vi "温度控制 - WK1.vi"(7 "CSM Name":string="WK1") -> ()   [LabVIEW 2026, in "UI-温度控制.lvlib"]
doc: "本范例执行串口读写操作。串口设置的参数必须匹配连接仪器或设备的参数。“VISA配置串口”VI可设置配置参数。前面板显示的控件可用于配置基本参数，如波特率、数据位和校验。VI会将VISA资源名称传递至其他VI以便执行相关操作。“VISA写入”函数将发送一个命令至串行设备，“VISA读取”函数将返回基于该命令的数据。“VISA关闭”函数可关闭该串行设备的引用。关闭引用十分重要，否则可能导致无法通过该端口进行进一步通信。"
uses:
  Supports/Sample Settings.ctl
  Data ColndSave/Supports/Time and Data.ctl
  Supports/Device Info.ctl
  Supports/Repeat Steps.ctl
  <userlib>/_NEVSTOP/Communicable State Machine(CSM)/_Polymophic/CSM - Filter Duplicated Lines.vi
  <userlib>/_NEVSTOP/Communicable State Machine(CSM)/_Polymophic/Add State(s) to Queue By BOOL(Element).vi
  e87f5527-76ec-45cd-8a15-2e3ba2958834.vi
  e40b3fcb-6c9f-41ae-97ff-bcb9991e0652.vi
  620e82e9-b677-4d25-b56c-4b090e123e3d.vi
  fecb341a-c865-4baa-9917-6b90415d6ef9.vi
  afd7753c-ea30-4e5b-9716-29bc73ab5d02.vi
  9a199716-2ffa-4f43-b9de-bb583d0dc84c.vi
  b5fe0464-1048-4df8-950b-6816aac68042.vi
  026bd4a5-6a46-4a68-819b-9f168641a175.vi
  3bdb7142-561a-47bb-abd8-0318bec92597.vi
  36fd150c-2ad9-4592-a276-8ca334c7aa56.vi
  6094d1ba-01c9-4f0f-81c2-2bfc5faa83cd.vi
  6f01d93e-47d7-4c16-bfcb-79e48a01ebec.vi
  f347ec19-a9ab-456c-bf02-8d1d7c992b68.vi
  b7989555-3743-433e-92bc-1f24cc67f5f4.vi
  9b669b8c-733c-4058-8ee2-0fdaa3bce225.vi
  7ceba0d5-fd35-45f6-9e4f-db13be910fa9.vi
  e0d25892-2f3c-4bdd-91b3-ce78b04bde2a.vi
  e709ab76-91cd-483a-bfeb-5221a7f7e432.vi
  6fdd3ccc-b7af-4740-b642-363912b39baa.vi
  52a88361-96b9-4f42-83b5-2b3a91f6fe46.vi
  <userlib>/_NEVSTOP/Communicable State Machine(CSM)/_Polymophic/CSM - Replace Marks in Messages.vi
  3eee923a-0692-424c-8c25-dbf31775acba.vi
  7f493404-46e2-4a42-937c-85a599ffd008.vi
  e181f527-371e-42fd-b1ab-20e25477ecf6.vi
  3c0606d2-39f9-4349-a74d-1248628ec5a5.vi
  2a5f06fa-bc14-4be7-8a56-d3603e987429.vi
  b1075206-a0bc-4c2c-8117-03daddfb89bc.vi
  f1339c31-251d-401b-9b2c-5eea904d101d.vi
  12798cb0-d503-413b-8ceb-4a5576430bcb.vi
  342b248c-6441-4aa8-8129-3c8b576c20b5.vi
  bd3fa8c0-2a07-4348-928a-5492c50b8d1d.vi
  bfd69444-e477-482d-b4ce-b6780147d2f5.vi
  22b4bb12-f94e-4276-9d0b-49463fdbebaf.vi
  87263e8e-d87a-4015-b0d9-f89f6746087b.vi
  45ac6a38-59b2-4408-864e-de2893445c95.vi
  3f8d9458-3e99-4457-8efa-55d1ef2330f2.vi
  bd3177e1-6bd6-42ad-a258-ed35146a2f34.vi
  acea6df9-f425-4d5c-b033-3243991d638c.vi
  611bdd8b-2aca-4a53-81a9-536b5b4081e0.vi
  6c66f1b3-0c4e-481a-bccf-761e4204c7a2.vi
  69110340-9523-4369-a866-1e083b49cebd.vi
  dc7ef564-96da-43a3-866d-645d9c897f58.vi
  cab45986-ae3d-44a0-b15a-916822da0a04.vi
  6e92e572-67e2-4f23-93e9-3f2621f8ebb2.vi
  fcc43e12-244c-4800-bcec-4b40395c6c4b.vi
  b77c82fb-bb1b-4fca-94e8-a2470f067fd9.vi
  <userlib>/_NEVSTOP/Communicable State Machine(CSM)/AdvanceAPI/CSM - Compact Multiple States.vi
  <userlib>/_NEVSTOP/Communicable State Machine(CSM)/AdvanceAPI/CSM - Break Down Multiple States String.vi
  <userlib>/_NEVSTOP/Communicable State Machine(CSM)/_Shared/Remove Comments from Single-line.vi
  <userlib>/_NEVSTOP/Communicable State Machine(CSM)/_Shared/Split Single-line Message.vi
  <userlib>/_NEVSTOP/Communicable State Machine(CSM)/_Shared/Trim Single-line Text.vi
  <userlib>/_NEVSTOP/Communicable State Machine(CSM)/_Shared/Add State(s) to Queue__jkism.vi
  <userlib>/_NEVSTOP/Communicable State Machine(CSM)/AdvanceAPI/CSM - Revert Arguments-Safe String.vi
  <userlib>/_NEVSTOP/Communicable State Machine(CSM)/AdvanceAPI/CSM - Make String Arguments Safe.vi
  e709ab76-91cd-483a-bfeb-5221a7f7e432.vi/99de0c97-112a-4c86-9094-c187659127e1.vi
  <userlib>/_NEVSTOP/Communicable State Machine(CSM)/Utility/Build Error Cluster.vi
  52a88361-96b9-4f42-83b5-2b3a91f6fe46.vi/99de0c97-112a-4c86-9094-c187659127e1.vi
  cab45986-ae3d-44a0-b15a-916822da0a04.vi/b09b9099-6be0-413b-8afc-4908471460c3.vi
  <userlib>/_NEVSTOP/Communicable State Machine(CSM)/addons/INI-Static-Variable-Support/_Support/FlagInstance-CSMINIVariable.vi
  b77c82fb-bb1b-4fca-94e8-a2470f067fd9.vi/99de0c97-112a-4c86-9094-c187659127e1.vi
  <vilib>/Utility/error.llb/Trim Whitespace.vi
  <vilib>/Utility/error.llb/Trim Whitespace (string).vi
  <userlib>/_NEVSTOP/Communicable State Machine(CSM)/AdvanceAPI/CSM - Keywords.vi
  <userlib>/_NEVSTOP/Communicable State Machine(CSM)/_Support/ChangeFlag/ChangeFlag-Read.vi
  <vilib>/Utility/error.llb/Trim Whitespace One-Sided.vi
  <userlib>/_NEVSTOP/Communicable State Machine(CSM)/addons/API-String-Arugments-Support/_Support/Data To API String Arguments.vi
  <userlib>/_NEVSTOP/Communicable State Machine(CSM)/addons/INI-Static-Variable-Support/_Support/instances/_CSM - Read File Logger Configuration - v1.0.vi
  <vilib>/Utility/Data Type/Get Type Information.vi
  <userlib>/_NEVSTOP/Communicable State Machine(CSM)/addons/API-String-Arugments-Support/_Support/Data To SingleElementsArray_csm.vi
  <userlib>/_NEVSTOP/Communicable State Machine(CSM)/addons/INI-Static-Variable-Support/_Support/Parse Used Session and Name.vi
  <userlib>/_NEVSTOP/Communicable State Machine(CSM)/addons/INI-Static-Variable-Support/_Support/INI-FGV(lvlibp).vi
  <userlib>/_NEVSTOP/Communicable State Machine(CSM)/addons/INI-Static-Variable-Support/_Support/Populate String with INI Variable.vi
  <userlib>/_NEVSTOP/Communicable State Machine(CSM)/addons/API-String-Arugments-Support/_Support/Convert API String Arguments to Data(variant).vi
  <userlib>/_NEVSTOP/Communicable State Machine(CSM)/addons/API-String-Arugments-Support/_Support/SingleElementsArray To Data_csm.vi
  <userlib>/_NEVSTOP/Communicable State Machine(CSM)/addons/MassData-Parameter/_support/FGV-MassData(lvlibp).vi
  <vilib>/Instr/_visa.llb/VISA Configure Serial Port (Instr).vi
  Repeat/Repeat.vi
  <userlib>/_NEVSTOP/Communicable State Machine(CSM)/_Support/ChangeFlag/ChangeFlagDB.vi
  <userlib>/_NEVSTOP/Communicable State Machine(CSM)/Communicable State Machine.lvlib
  <userlib>/_NEVSTOP/Communicable State Machine(CSM)/addons/MassData-Parameter/CSM MassData Parameter Support.lvlib
  <userlib>/_NEVSTOP/Communicable State Machine(CSM)/addons/INI-Static-Variable-Support/INI-Static-Variable-Support.lvlib
  <userlib>/_NEVSTOP/Communicable State Machine(CSM)/addons/Watchdog/CSM Watchdog.lvlib
  <userlib>/_NEVSTOP/Communicable State Machine(CSM)/addons/Logger/CSM File Logger.lvlib
  Logging/Logging.lvlib
  Repeat/Repeat.lvlib
  b63380f4-522f-43f9-8c86-ff87e18121f1.vi
  Acquisition/Acquisition.lvlib
  Data ColndSave/Data Collection and Save.lvlib
panel:
  in  "停止":bool
  in  "温度显示":T1(tab)
  in  "下限 2":dbl=25.0 min=-10.0 max=50.0 step=0.1 format="%.1g"
  in  "上限 2":dbl=25.0 min=-10.0 max=50.0 step=0.1 format="%.1g"
  in  "下限 1":dbl=25.0 min=-10.0 max=50.0 step=0.1 format="%.1g"
  in  "上限 1":dbl=25.0 min=-10.0 max=50.0 step=0.1 format="%.1g"
  in  "温控开关 总":bool
  in  "跟随通道 1":T2
  in  "跟随通道 2":T2
  in  "通道":bool
  in  "温控温度 B":dbl=25.0 min=-10.0 max=50.0 step=0.1 format="%.2g"
  in  "温控温度 A":dbl=25.0 min=-10.0 max=50.0 step=0.1 format="%.2g"
  in  "温度":bool
  in  "跟随偏移 2":dbl min=-10.0 max=50.0 step=0.01 format="%#.2g"
  in  "是否跟随 2":bool
  in  "跟随偏移 1":dbl min=-10.0 max=50.0 step=0.01 format="%#.2g"
  in  "是否跟随 1":bool
  in  "打开串口":bool
  in  "温控串口":refnum<visa-resource-name>="COM18"
  out "TC2":waveform(dbl)[](graph)
  out "TC1":waveform(dbl)[](graph)
  in  "温控开关 2":bool
  in  "温控开关 1":bool
  in  "温控温度 2":dbl=25.0 min=-10.0 max=50.0 step=0.1 format="%.2g"
  out "实际温度 2":dbl=25.0 format="%.2g"
  out "实际温度 1":dbl=25.0 format="%.2g"
  in  "温控温度 1":dbl=25.0 min=-10.0 max=50.0 step=0.1 format="%.2g"
  in  "Fast Mode":bool
  in  "采集间隔":dbl=0.5 min=0.05 max=50.0 step=0.1 format="%.2g"
  out "Power 2":waveform(dbl)[](graph)
  out "Power 1":waveform(dbl)[](graph)
  out "输出状态 1":T3
  out "输出状态 2":T3
  in  "电源切换 2":bool
  in  "电源切换 1":bool
  in  "输出设置 2":T4={"输出模式"=enum."加热模式", "最大输出电压"=5.0} {"最大输出电压" min=0.0001 max=10.0 format="%.1g"}
  in  "输出设置 1":T4={"输出模式"=enum."加热模式", "最大输出电压"=5.0} {"最大输出电压" min=0.0001 max=10.0 format="%.1g"}
  in  "PID 1":T5={"PID类型"=enum."PID", "P"=0.05, "I"=20.0, "D"=2.0, "PID控制间隔"=100.0, "PID计算方法"=enum."最大正向输出"}
  in  "PID 2":T5={"PID类型"=enum."PID", "P"=0.05, "I"=20.0, "D"=2.0, "PID控制间隔"=100.0, "PID计算方法"=enum."最大正向输出"}
  in  "过压/过流 2":cluster{"过压保护阈值":dbl, "过流保护阈值":dbl}={"过压保护阈值"=6.0, "过流保护阈值"=3.0}
  in  "过压/过流 1":cluster{"过压保护阈值":dbl, "过流保护阈值":dbl}={"过压保护阈值"=6.0, "过流保护阈值"=3.0}
  in  "过温 2":T6={"过温保护开关"=TRUE, "过温保护低阈值"=5.0, "过温保护高阈值"=45.0, "最低设定温度"=5.0, "最高设定温度"=45.0, "温度限速"=45.0} {"温度限速" min=0.01}
  out "保护结果 2":T7={"过压保护结果"=enum."正常", "过流保护结果"=enum."正常", "过温保护结果"=enum."正常"}
  out "保护结果 1":T7={"过压保护结果"=enum."正常", "过流保护结果"=enum."正常", "过温保护结果"=enum."正常"}
  in  "过温 1":T6={"过温保护开关"=TRUE, "过温保护低阈值"=5.0, "过温保护高阈值"=45.0, "最低设定温度"=5.0, "最高设定温度"=45.0, "温度限速"=45.0} {"温度限速" min=1e-06; "最低设定温度" min=0.0001}
  in  "温控循环功能":bool
  in  "子程序？":bool
  out "温控-错误输出":errorcluster
  out "温控器设备型号":string
  out "State History":string
  # "温度快切"
  # "V"
  # "A"
  # "V"
  # "A"
  # "V"
  # "V"
  # "ms"
  # "ms"
  # "℃/s"
  # "℃/s"
  # "恢复，继续运行；\n如继续报错，请检查参数，可尝试关闭串口重新打开。"
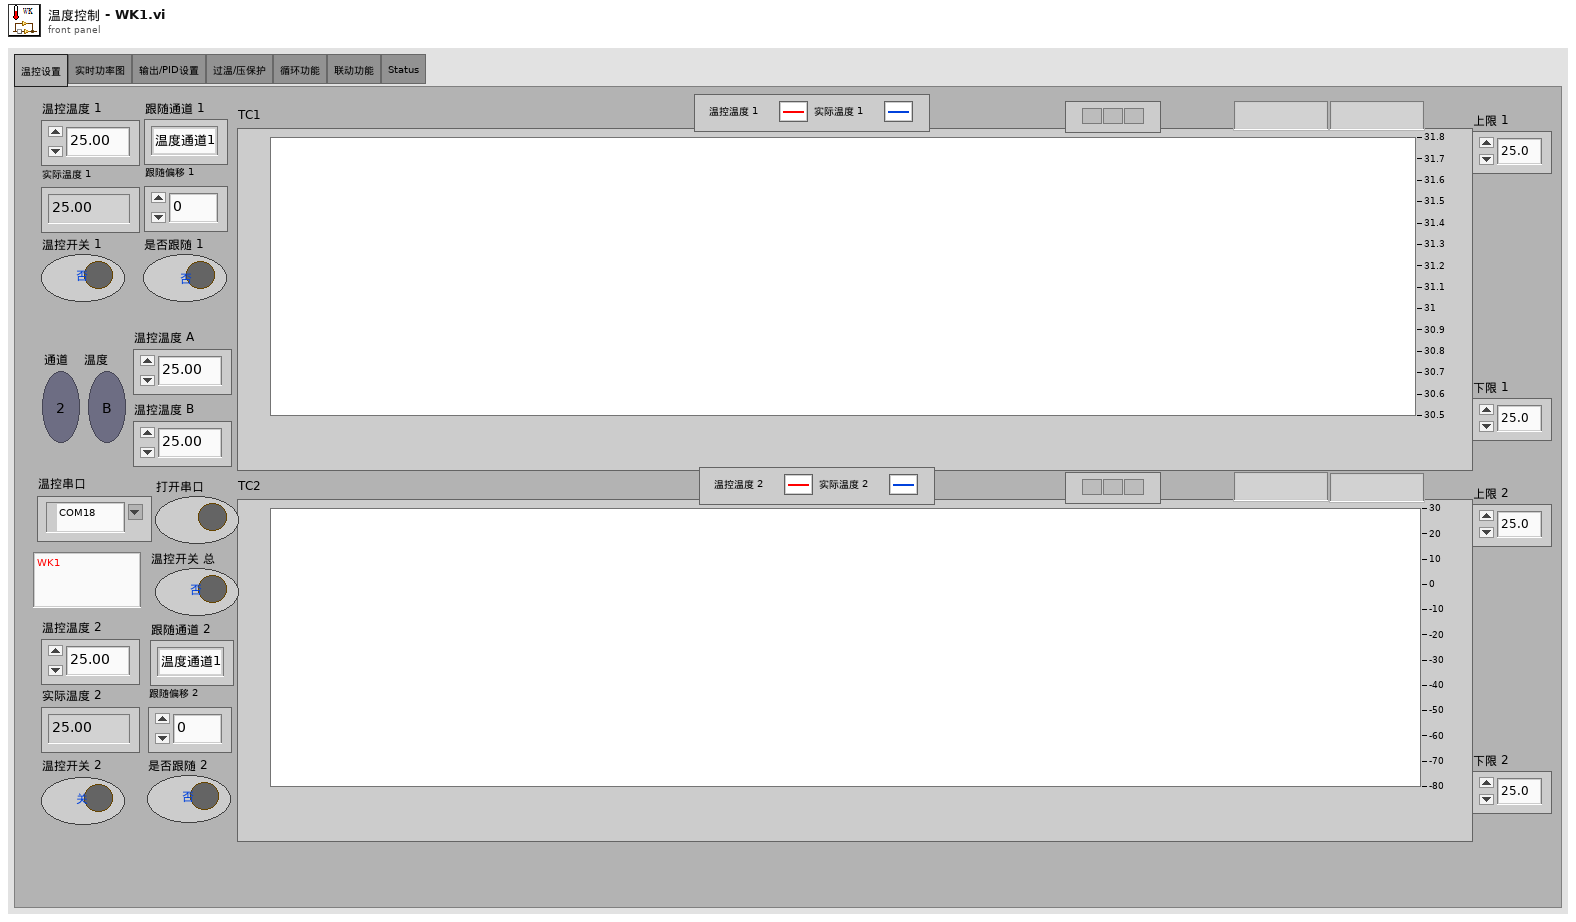
[diagram p1: front panel]
types:
  T1 = enum32{"温控设置", "实时功率图", "输出/PID设置", "过温/压保护", "循环功能", "联动功能", "Status"}
  T2 = typedef "温度通道索引_全局.ctl" = enum16{"温度通道1", "温度通道2", "温度通道3", "温度通道4", "温度通道5", "温度通道6", "温度通道7", "温度通道8", "TC1控制温度", "TC1实际温度", "TC1实际输出电压", "TC1实际输出电流", "TC1实际输出功率", "TC2控制温度", "TC2实际温度", "TC2实际输出电压", "TC2实际输出电流", "TC2实际输出功率", "压力(电压值)", "压力(g)", "Zolix当前位置", "Zolix速度", "步进电机位置", "步进电机速度", "温度", "湿度"}
  T3 = cluster{"功率输出":enum16{"已关闭", "已打开"}, "实际输出电压":dbl, "实际输出电流":dbl}
  T4 = cluster{"输出模式":enum16{"致冷模式", "加热模式", "双向模式"}, "最大输出电压":dbl}
  T5 = cluster{"PID类型":enum16{"P", "PI", "PID"}, "P":dbl, "I":dbl, "D":dbl, "PID控制间隔":dbl, "PID计算方法":enum16{"位置式", "增量式", "最大正向输出", "最大负向输出"}}
  T6 = cluster{"过温保护开关":bool, "过温保护低阈值":dbl, "过温保护高阈值":dbl, "最低设定温度":dbl, "最高设定温度":dbl, "温度限速":dbl}
  T7 = cluster{"过压保护结果":enum16{"发现错误", "正常", "功能关闭"}, "过流保护结果":enum16{"发现错误", "正常", "功能关闭"}, "过温保护结果":enum16{"发现错误", "正常", "功能关闭"}}
  T8 = cluster{"Enable":bool, "Limit":cluster{"FileSize":i64, "FileNum":i32}, "Timestamp.Format":string, "AutoExit":bool}
  T9 = enum32{"Invalid", "Standard", "Closed", "Hidden", "Minimized", "Maximized"}
  T10 = enum32{"invalid app kind", "Development System", "Run Time System", "Student Edition", "Embedded LabVIEW", "Evaluation", "Custom"}
  T11 = typedef "UI-温度控制.lvlib/Device Info.ctl" = cluster{"基本信息":cluster{"USB Port":refnum<visa-resource-name>, "采集间隔(s)":dbl}, "设备信息":cluster{"设备型号":string, "双通道设备？":bool}, "开关":cluster{"开关 1":bool, "开关 2":bool, "Fast Mode":bool}, "Control Temp":cluster{"Control Temp 1":dbl, "Control Temp 2":dbl}}
  T12 = cluster{"波特率":u32, "数据位":u16, "校验":enum16{"None", "Odd", "Even", "Mark", "Space"}, "停止位":u16, "流控制":u16}
  T13 = typedef "Communicable State Machine.lvlib/_CSM_Response Source Message.ctl" = cluster{"‘State":string, "’Arguments":string, "’Error":errorcluster}
  T14 = cluster{"Current VI Reference":refnum<vi>, "Close Panel on Exit?":bool}
  T15 = typedef "UI-温度控制.lvlib/Sample Settings.ctl" = cluster{"USB Port":refnum<visa-resource-name>, "采集间隔(s)":dbl}
  T16 = typedef "Data Collection and Save.lvlib/Time and Data.ctl" = cluster{"采集时间":timestamp, "Data":dbl[]}
  T17 = cluster{"Core":cluster{"Current VI Reference":refnum<vi>, "Close Panel on Exit?":bool}, "基本信息":T15, "温控情况":cluster{"温控温度 1":dbl, "实际温度 1":dbl, "温控温度 2":dbl, "实际温度 2":dbl, "打开串口":bool}, "开关信息":cluster{"开关 1":bool, "开关 2":bool, "温控是否打开":bool}, "输出参数":cluster{"输出设置 1":cluster{"输出模式":enum16{"致冷模式", "加热模式", "双向模式"}, "最大输出电压":dbl}, "输出设置 2":cluster{"输出模式":enum16{"致冷模式", "加热模式", "双向模式"}, "最大输出电压":dbl}, "输出状态 1":cluster{"功率输出":enum16{"已关闭", "已打开"}, "实际输出电压":dbl, "实际输出电流":dbl, "实际输出功率":dbl}, "输出状态 2":cluster{"功率输出":enum16{"已关闭", "已打开"}, "实际输出电压":dbl, "实际输出电流":dbl, "实际输出功率":dbl}, "PID 1":cluster{"PID类型":enum16{"P", "PI", "PID"}, "P":dbl, "I":dbl, "D":dbl, "PID控制间隔":dbl, "PID计算方法":enum16{"位置式", "增量式", "最大正向输出", "最大负向输出"}}, "PID 2":cluster{"PID类型":enum16{"P", "PI", "PID"}, "P":dbl, "I":dbl, "D":dbl, "PID控制间隔":dbl, "PID计算方法":enum16{"位置式", "增量式", "最大正向输出", "最大负向输出"}}}, "保护":cluster{"过压/过流 1":cluster{"过压保护阈值":dbl, "过流保护阈值":dbl}, "过压/过流 2":cluster{"过压保护阈值":dbl, "过流保护阈值":dbl}, "保护结果 1":cluster{"过压保护结果":enum16{"发现错误", "正常", "功能关闭"}, "过流保护结果":enum16{"发现错误", "正常", "功能关闭"}, "过温保护结果":enum16{"发现错误", "正常", "功能关闭"}}, "保护结果 2":cluster{"过压保护结果":enum16{"发现错误", "正常", "功能关闭"}, "过流保护结果":enum16{"发现错误", "正常", "功能关闭"}, "过温保护结果":enum16{"发现错误", "正常", "功能关闭"}}, "过温 1":cluster{"过温保护开关":bool, "过温保护低阈值":dbl, "过温保护高阈值":dbl, "最低设定温度":dbl, "最高设定温度":dbl, "温度限速":dbl}, "过温 2":cluster{"过温保护开关":bool, "过温保护低阈值":dbl, "过温保护高阈值":dbl, "最低设定温度":dbl, "最高设定温度":dbl, "温度限速":dbl}}, "设备信息":cluster{"设备型号":string, "双通道设备？":bool}, "Time and Data":T16, "其他":cluster{"子程序？":bool, "Fast Mode?":bool, "Auto Range 1?":bool, "Auto Range 2?":bool}}
  T18 = cluster{"子程序？":bool, "Fast Mode?":bool, "Auto Range 1?":bool, "Auto Range 2?":bool}
  T19 = cluster{"过压/过流 1":cluster{"过压保护阈值":dbl, "过流保护阈值":dbl}, "过压/过流 2":cluster{"过压保护阈值":dbl, "过流保护阈值":dbl}, "保护结果 1":cluster{"过压保护结果":enum16{"发现错误", "正常", "功能关闭"}, "过流保护结果":enum16{"发现错误", "正常", "功能关闭"}, "过温保护结果":enum16{"发现错误", "正常", "功能关闭"}}, "保护结果 2":cluster{"过压保护结果":enum16{"发现错误", "正常", "功能关闭"}, "过流保护结果":enum16{"发现错误", "正常", "功能关闭"}, "过温保护结果":enum16{"发现错误", "正常", "功能关闭"}}, "过温 1":cluster{"过温保护开关":bool, "过温保护低阈值":dbl, "过温保护高阈值":dbl, "最低设定温度":dbl, "最高设定温度":dbl, "温度限速":dbl}, "过温 2":cluster{"过温保护开关":bool, "过温保护低阈值":dbl, "过温保护高阈值":dbl, "最低设定温度":dbl, "最高设定温度":dbl, "温度限速":dbl}}
  T20 = cluster{"输出设置 1":cluster{"输出模式":enum16{"致冷模式", "加热模式", "双向模式"}, "最大输出电压":dbl}, "输出设置 2":cluster{"输出模式":enum16{"致冷模式", "加热模式", "双向模式"}, "最大输出电压":dbl}, "输出状态 1":cluster{"功率输出":enum16{"已关闭", "已打开"}, "实际输出电压":dbl, "实际输出电流":dbl, "实际输出功率":dbl}, "输出状态 2":cluster{"功率输出":enum16{"已关闭", "已打开"}, "实际输出电压":dbl, "实际输出电流":dbl, "实际输出功率":dbl}, "PID 1":cluster{"PID类型":enum16{"P", "PI", "PID"}, "P":dbl, "I":dbl, "D":dbl, "PID控制间隔":dbl, "PID计算方法":enum16{"位置式", "增量式", "最大正向输出", "最大负向输出"}}, "PID 2":cluster{"PID类型":enum16{"P", "PI", "PID"}, "P":dbl, "I":dbl, "D":dbl, "PID控制间隔":dbl, "PID计算方法":enum16{"位置式", "增量式", "最大正向输出", "最大负向输出"}}}
  T21 = cluster{"温控温度 1":dbl, "实际温度 1":dbl, "温控温度 2":dbl, "实际温度 2":dbl, "打开串口":bool}
  T22 = enum8{"Enabled", "Disabled", "Disabled and Grayed Out"}
  T23 = typedef "UI-温度控制.lvlib/Repeat Steps.ctl" = cluster{"控制温度":dbl, "时长(s)":dbl, "进度":dbl, "温控开关":bool}[]
  T24 = cluster{"PID类型":bool, "P":bool, "I":bool, "D":bool, "PID控制间隔":bool, "PID计算方法":bool}
  T25 = cluster{"过温保护开关":bool, "过温保护低阈值":bool, "过温保护高阈值":bool, "最低设定温度":bool, "最高设定温度":bool, "温度限速":bool}
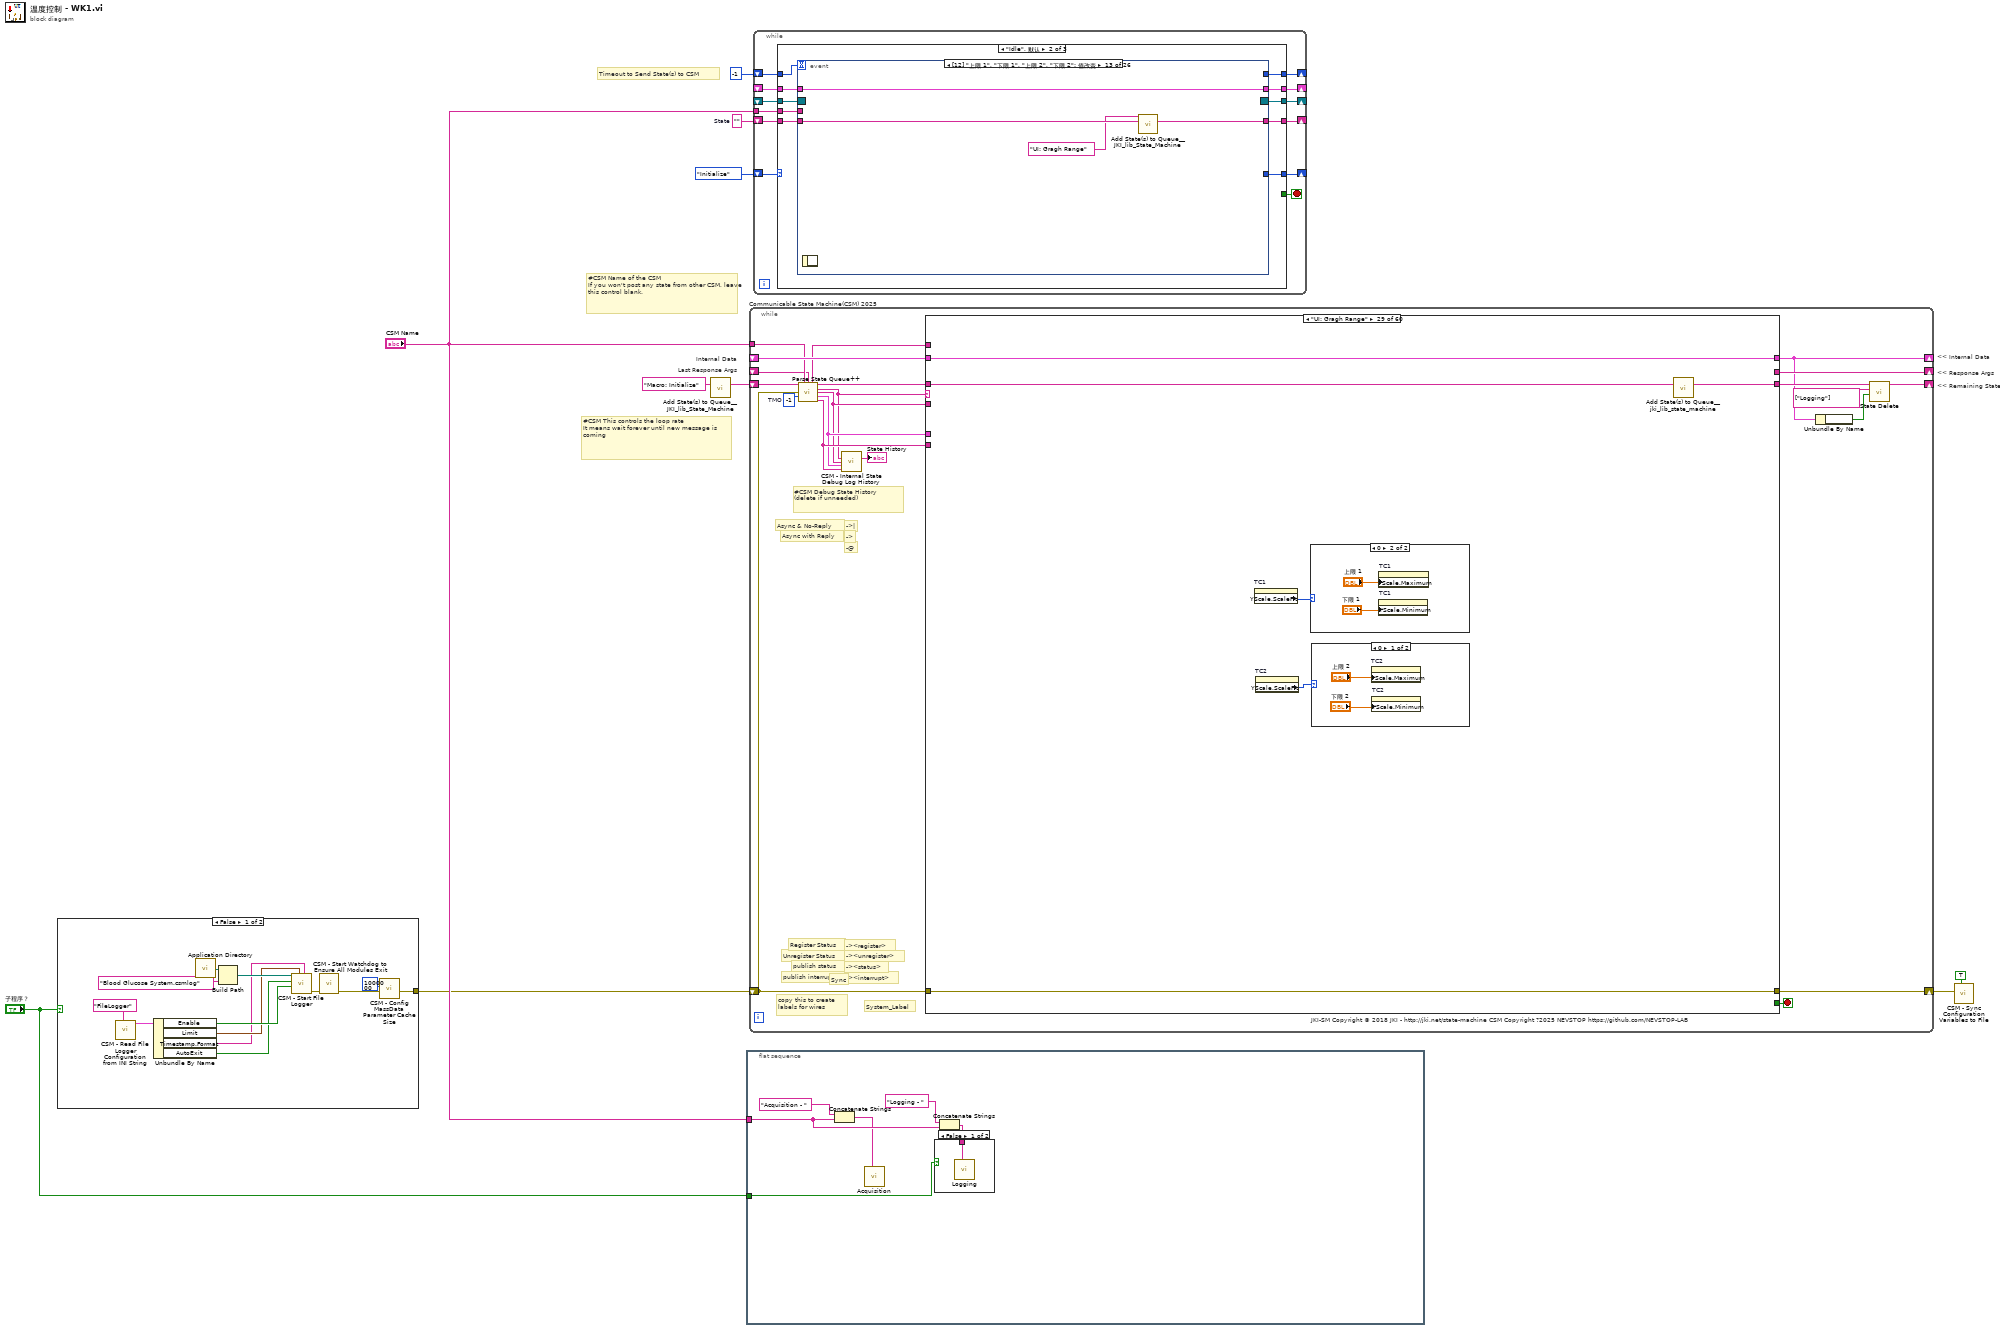
[diagram p0: block diagram]
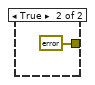
[diagram p2: hidden frame]
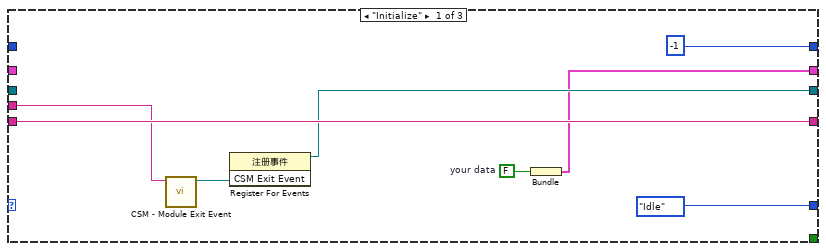
[diagram p4: hidden frame]
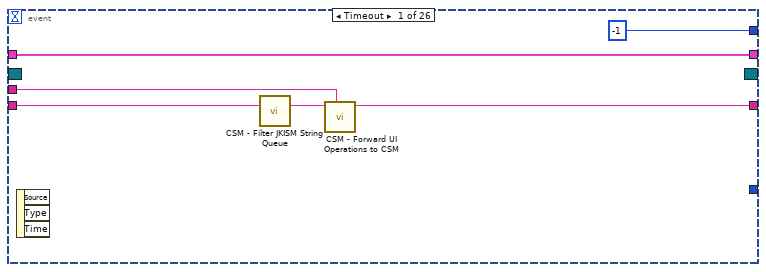
[diagram p5: hidden frame]
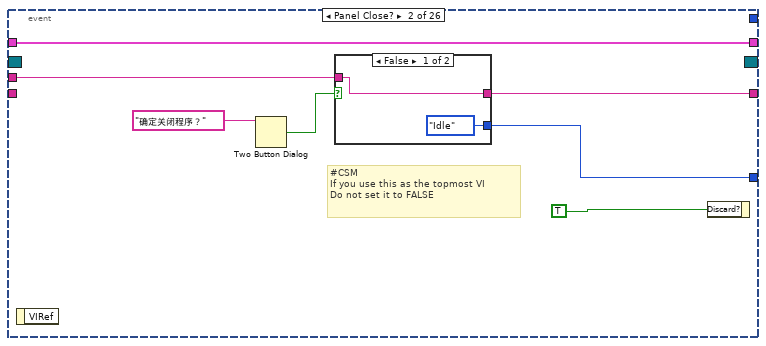
[diagram p6: hidden frame]
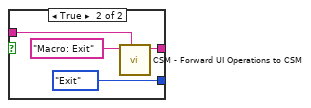
[diagram p7: hidden frame]
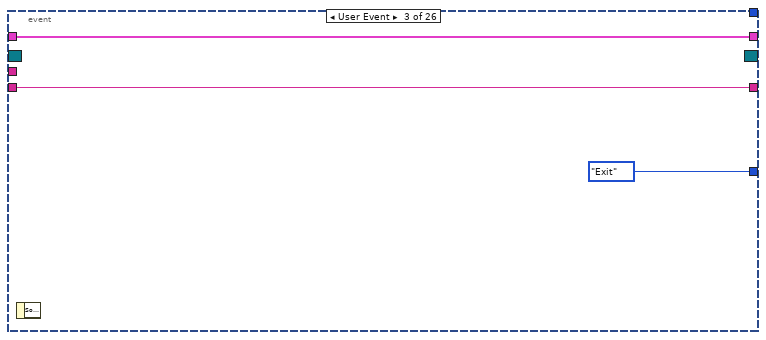
[diagram p8: hidden frame]
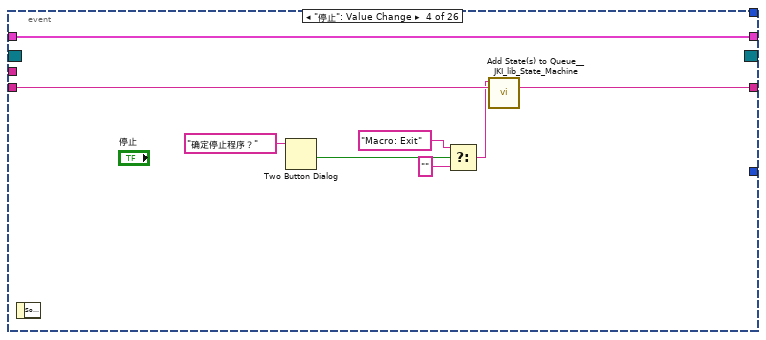
[diagram p9: hidden frame]
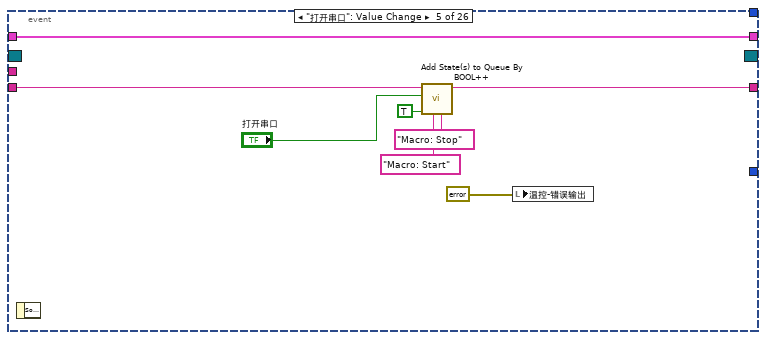
[diagram p10: hidden frame]
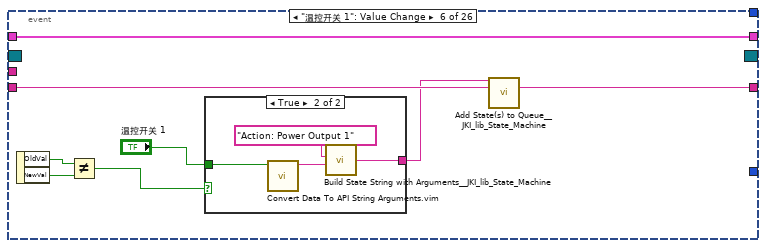
[diagram p11: hidden frame]
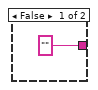
[diagram p12: hidden frame]
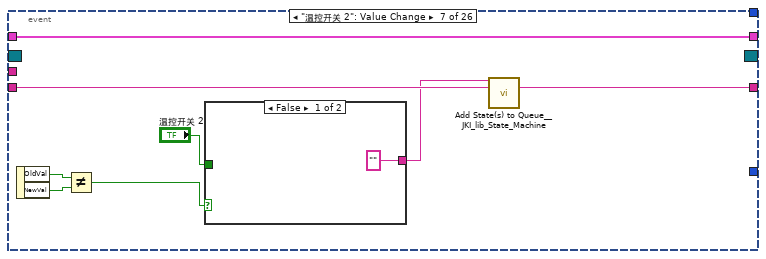
[diagram p13: hidden frame]
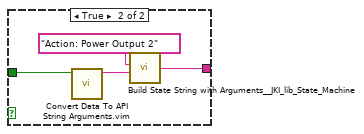
[diagram p14: hidden frame]
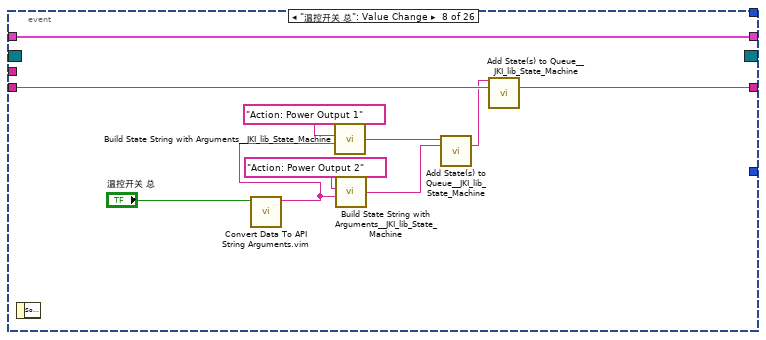
[diagram p15: hidden frame]
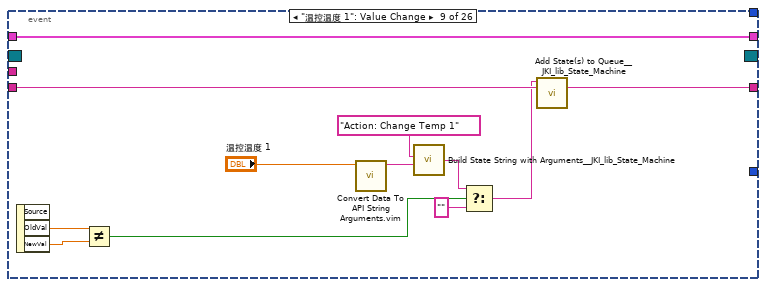
[diagram p16: hidden frame]
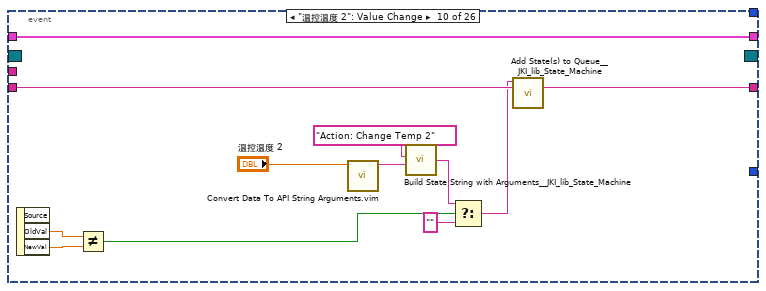
[diagram p17: hidden frame]
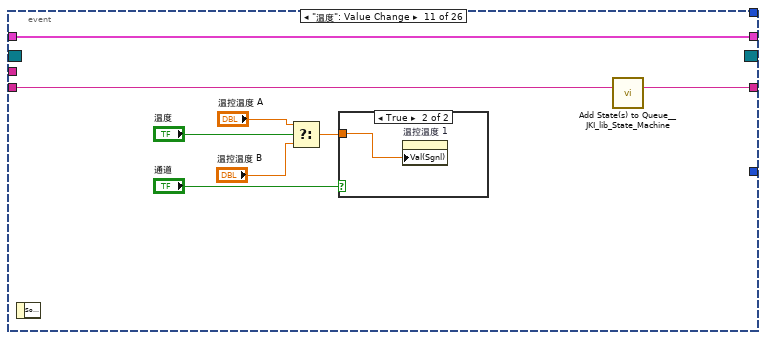
[diagram p18: hidden frame]
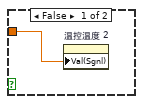
[diagram p19: hidden frame]
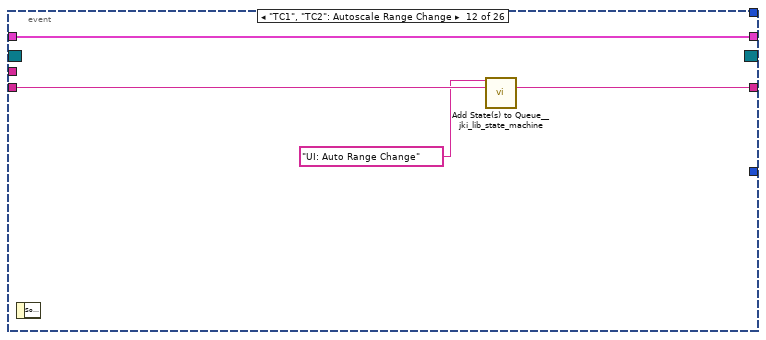
[diagram p20: hidden frame]
diagram:
  w9 = ""  # State
  # "Timeout to Send State(s) to CSM"
  # "Last Response Args"
  # "Internal Data"
  # "#CSM Name of the CSM\nIf you won't post any state from other CSM, leave this control blank."
  # "#CSM This controls the loop rate\nIt means wait forever until new message is coming"
  # "<< Internal Data"
  # "<< Response Args"
  # "<< Remaining States"
  n1 = case shown="False" "子程序？" {
    tunnel: [w21 errorcluster {"status"=FALSE, "code"=0, "source"=""} ("Error out")] -> w2
    frame False {
      n2 = call-poly <userlib>:"CSM - Read File Logger Configuration from INI String.vi"("Section Name(\"FileLogger\")"="FileLogger" ("Section Name(\"\" as Default)")) -> ("FileLogger Configuration-v1"=w15:T8)  [unwired: 7 in, 1 out]
      n3 = Unbundle By Name(w15) -> ("Enable"=w14:bool, "Limit"=w13:cluster{"FileSize":i64, "FileNum":i32}, "Timestamp.Format"=w11:string, "AutoExit"=w12:bool)
      n4 = call <vilib>:"Application Directory.vi"() -> ("Application Directory"=w20:path)
      n5 = Build Path(base path=w20, name or relative path="Blood Glucose System.csmlog") -> (appended path=w18:path)
      n6 = call <userlib>:"CSM - Start File Logger.vi"("Timestamp Format"=w11, "Log Limit"=w13, "Watchdog? (T)"=w14, "Exit When All Module Exist? (F)"=w12, "Log File Path"=w18) -> ("error out"=w17:errorcluster)  [unwired: 4 in, 2 out]
      n7 = call <userlib>:"CSM - Start Watchdog to Ensure All Modules Exit.vi"("error in (no error)"=w17) -> ("error out"=w22:errorcluster)  [unwired: 10 in]
      n8 = call <userlib>:"CSM - Config MassData Parameter Cache Size.vi"("Error in"=w22, "Size (50M)"=1000000 ("size(1M)")) -> ("Error out"=w21:errorcluster)  [unwired: 9 in]
    }
    frame True {
    }
  }
  n9 = call <vilib>:"Add State(s) to Queue__JKI_lib_State_Machine.vi"("State(s) in (\"\")"="Macro: Initialize" ("Init State(\"Macro: Initialize\")")) -> ("States Out"=w6:string)  [unwired: 14 in]
  n10 = flat-sequence {
    tunnel: "CSM Name" -> [w27]
    tunnel: "子程序？" -> [w25]
    frame #0 {
      n11 = Concatenate Strings("Acquisition - " ("Name(\"\" to use uuid)"), w27) -> (w26:string)
      n12 = call "Acquisition.vi"("CSM Name"=w26) -> ()  [unwired: 11 in]
      n13 = Concatenate Strings("Logging - " ("Name(\"\" to use uuid)"), w27) -> (w28:string)
      n14 = case shown="False" w25 {
        tunnel: w28 -> [w31 _]
        frame False {
          n15 = call "Logging.vi"("CSM Name"=w31) -> ()  [unwired: 11 in]
        }
        frame True {
        }
      }
    }
  }
  n16 = while "Communicable State Machine(CSM) 2025" {
    shift-right: [w33] -> _
    shift-left: _ -> [w48]
    shift-right: [w50] -> w4
    shift-left: w2 -> [w39]
    shift-right: [w35] -> _
    shift-left: w6 -> [w51]
    tunnel: "CSM Name" -> [w45]
    shift-right: [w46] -> _
    shift-left: _ -> [w40]
    stop <- w49 stop-if-true
    w47 = -1  # TMO
    # "#CSM Debug State History\n(delete if unneeded)"
    # "-><interrupt>"
    # "-><status>"
    # "-><unregister>"
    # "-><register>"
    # "-@"
    # "->"
    # "->|"
    # "publish interrupt"
    # "publish status"
    # "Unregister Status"
    # "Register Status"
    # "Sync"
    # "Async with Reply"
    # "Async & No-Reply"
    # "JKI-SM Copyright © 2018 JKI - http://jki.net/state-machine CSM Copyright ?2025 NEVSTOP https://github.com/NEVSTOP-LAB"
    # "copy this to create labels for wires"
    # "System_Label"
    n17 = call <userlib>:"Parse State Queue++.vi"("State Queue"=w51, "Name (\"\" to Use UUID)"=w45, "Response Arguments"=w40, "Previous Error"=w39, "Dequeue (1 ms)"=w47) -> ("Name Used"=w37:string, "Remaining States"=w52:string, "Current State"=w41:string, "Arguments"=w42:string, "Additional Information"=w43:T13, "Source CSM"=w44:string)  [unwired: 5 in]
    n18 = call <userlib>:"CSM - Internal State Debug Log History.vi"("State"=w41, "Arguments (\"\")"=w42, ">> Response Source Message >>"=w43, "Source (\"\")"=w44) -> ("Debug Log"=→"State History":string)  [unwired: 11 in]
    n19 = case shown="\"UI: Gragh Range\"" w41 {
      selector: w41 -> [_ _ _ w64 _ _ _ _ _ _ _ _ _ _ _ _ _ _ _ _ _ _ _ _ _ _ _ _ _ _ _ _ _ _ _ _ _ _ _ _ _ _ _ _ _ _ _ _ _ _ _ _ _ _ _ _ _ _ _ _]
      tunnel: w52 -> [w53 w57 w60 w68 w73 w79 w104 w110 w116 w126 w133 w145 w149 w152 w172 w212 w238 w240 w261 w263 w295 w321 w352 w383 w440 w514 w546 w553 w558 w567 w573 w619 w632 w661 w673 w676 w694 w712 w737 w749 w788 w803 w812 w839 w869 w914 w959 w1005 w1051 w1080 w1099 w1106 w1112 w1120 w1133 w1140 w1153 w1166 w1178 w1183]
      tunnel: w42 -> [_ _ _ _ _ w78 w100 w107 w113 w120 _ _ _ _ _ w205 _ _ _ _ _ _ _ _ _ _ _ _ _ _ _ _ _ _ _ _ w686 w704 w726 w743 w781 w796 w811 w838 w868 w913 w958 w1004 w1050 w1079 _ w1104 w1115 w1123 w1130 _ _ w1164 _ _]
      tunnel: w48 -> [w55 w56 w58 w66 w72 w84 w102 w108 w114 w124 w132 w139 w147 w150 _ w183 w233 w241 w245 w267 w286 w314 w326 w357 w417 w495 w516 w552 w557 w565 w571 w598 w620 w665 w669 w674 w683 w701 w729 w746 w778 w793 w807 w834 w862 w905 w951 w998 w1042 w1071 w1098 w1102 w1117 w1125 w1131 w1138 w1145 w1168 w1176 w1182]
      tunnel: [_ _ _ w61 w74 errorcluster {"status"=FALSE, "code"=0, "source"=""} ("error out") w97 w105 w111 w127 _ _ _ _ _ _ w234 w242 w262 w268 w274 w298 w323 w354 w386 w461 w547 w554 w560 _ _ w582 w629 w666 _ _ w681 w699 w727 w744 w776 w791 w804 w831 w863 w908 w953 w999 w1045 w1074 _ w1110 w1118 w1126 w1137 _ _ w1169 _ w1184] -> w50
      tunnel: w39 -> [_ _ _ w62 w74 w82 w98 w106 w112 _ _ _ _ _ _ _ w235 w242 w262 w268 w284 w299 w324 w355 w387 w462 w547 w554 w560 _ _ w582 w630 w666 _ _ w687 w705 w724 w742 w782 w797 w805 w832 w864 w909 w954 w1000 w1046 w1075 _ w1110 w1118 w1126 w1137 _ _ w1169 _ w1184]
      tunnel: [w54 w57 w59 w67 w73 w80 w103 w109 w115 w125 w133 w144 w148 w151 w171 w213 w237 w239 w260 w264 w296 w322 w353 w384 w441 w515 w545 w553 w559 w566 w572 w618 w631 w662 w672 w675 w693 w711 w736 w748 w787 w802 w813 w840 w870 w915 w960 w1006 w1052 w1081 w1099 w1107 w1113 w1121 w1134 w1139 w1152 w1167 w1177 w1183] -> w36
      tunnel: [_ _ _ _ _ _ TRUE _ _ _ _ _ TRUE _ _ _ _ _ _ _ _ _ _ _ _ _ _ _ _ _ _ _ _ _ _ _ _ _ _ _ _ _ _ _ _ _ _ _ _ _ _ _ _ _ _ _ _ _ _ _] -> w49
      tunnel: [w55 w56 w58 w66 w72 w84 w102 w108 w114 w123 w132 w143 w147 w150 w170 w182 w233 w241 w245 w267 w272 w313 w325 w382 w415 w494 w516 w552 w557 w565 w571 w592 w628 w665 w669 w674 w682 w700 w728 w745 w777 w792 w806 w833 w858 w904 w949 w994 w1043 w1072 w1098 w1100 w1117 w1125 w1127 w1138 w1145 w1168 w1176 w1182] -> w33
      tunnel: w44 -> [_ _ _ _ _ w77 _ _ _ w121 _ _ _ _ _ _ _ _ _ _ _ _ _ _ _ _ _ _ _ _ _ _ _ _ _ _ _ _ _ _ _ _ _ _ _ _ _ _ _ _ _ _ _ _ _ _ _ _ _ _]
      tunnel: w43 -> [_ _ _ _ _ w76 _ _ _ w122 _ _ _ _ _ _ _ _ _ _ _ _ _ _ _ _ _ _ _ _ _ _ _ _ _ _ _ _ _ _ _ _ _ _ _ _ _ _ _ _ _ _ _ _ _ _ _ _ _ _]
      tunnel: [_ _ _ "" w69 _ _ _ _ _ _ _ _ _ _ _ _ _ _ _ _ _ _ _ _ _ _ _ _ _ _ _ _ _ _ _ _ _ _ _ _ _ _ _ _ _ _ _ _ _ _ _ _ _ _ _ _ _ _ _] -> w46
      tunnel: w37 -> [_ _ _ w63 _ _ w99 _ _ _ _ _ _ _ w162 _ w231 _ _ _ _ _ _ _ _ _ _ _ _ _ w569 w593 _ w663 w671 _ _ _ w713 w738 _ _ _ _ _ _ _ _ _ _ _ w1108 w1114 w1122 w1135 _ w1141 w1162 w1175 _]
      frame "", "Idle" {
        # "#CSM \"Idle/Event Handler\"\nexecutes when the state queue is empty"
        n20 = call <vilib>:"Add State(s) to Queue__JKI_lib_State_Machine.vi"("State(s) in (\"\")"=w53) -> ("States Out"=w54:string)  [unwired: 14 in]
      }
      frame "CSM Documentation" {
        # "#CSM State Syntax\n\n// Comment line, all text to the right of “//” will be ignored\n// Local Message Example\nDoSth: DoA >> Arguments\n\n// Sync Call Example\nAPI: xxxx >> Arguments -@ TargetModule\n\n// Async Call Example\nAPI: xxxx >> Arguments -> TargetModule\n\n// Async Call without Reply Example\nAPI: xxxx >> Arguments ->| TargetModule\n\n// Broadcast normal status:\nStatus >> StatusArguments  -><status>\n\n// Broadcast Interrupt status:\nInterrupt >> StatusArguments  -><interrupt>\n\n// Register Source Module's status to Handler Module\nStatus@Source Module >> Handler Module@Handler Module -><register>\n\n// Unegister Source Module's status\nStatus@Source Module >> Handler Module -><unregister>"
        # "#CSM README FIRST\n\nCommunicable State Machine(CSM) is a LabVIEW application framework that builds upon JKI State Machine(JKISM). It follows the pattern of JKISM and extends the keywords to describe message communication between modules, including concepts such as Sync-Message, Async-Message, Subscription/Unsubscription of status - essential elements for creating reusable code modules. For more information, please visit the CSM wiki: https://nevstop-lab.github.io/CSM-Wiki/\n\nFor instructions on JKI State Machine, visit: \n    http://jki.net/state-machine/\nFor information about CSM, visit: \n    https://github.com/NEVSTOP-LAB"
        # "#CSM \"Documentation\"\nCase for holding CSM Documenation"
      }
      frame "---------- Core ----------" {
        # "#CSM \"Category Seperator\"\nDo not put any code in this frame."
        n21 = call <vilib>:"Add State(s) to Queue__JKI_lib_State_Machine.vi"("State(s) in (\"\")"=w60) -> ("States Out"=w59:string)  [unwired: 14 in]
      }
      frame Default {
        # "#CSM \"Default\"\nthis is used to capture unhandled states and typos"
        n22 = call <userlib>:"CSM Unhandled State Error.vi"("error in (no error)"=w62, "Undefined State"=w64, "CSM Name"=w63) -> ("error out"=w61:errorcluster)  [unwired: 8 in]
        n23 = call <vilib>:"Add State(s) to Queue__JKI_lib_State_Machine.vi"("State(s) in (\"\")"=w68) -> ("States Out"=w67:string)  [unwired: 14 in]
      }
      frame "VI Reference" {
        n24 = Unbundle By Name(w72) -> ("Core"=w71:T14)
        n25 = Unbundle By Name(w71) -> ("Current VI Reference"=w70:refnum<vi>)
        n26 = call <userlib>:"CSM - Convert Data to HexStr.vi"("Variant"=w70) -> ("HEX String (0-9,A-F)"=w69:string)  [unwired: 8 in]
      }
      frame "Error Handler" {
        # "#CSM \"Error Handler\"\nYou can also output any states to clean-up after errors occur"
        # "Clear error"
        n27 = case shown="无错误" w82 {
          selector: w82 -> [_ w91]
          tunnel: [w89 w93] -> w81
          tunnel: w79 -> [w89 w92]
          tunnel: w78 -> [w88 _]
          tunnel: w77 -> [_ _]
          tunnel: w76 -> [_ _]
          tunnel: [w86 w91] -> w75
          frame No Error {
            n28 = call <userlib>:"CSM - Convert Argument to Error.vi"("Argument"=w88) -> ("Error"=w87:errorcluster)  [unwired: 4 in]
            n29 = flat-sequence {
              tunnel: w87 -> [w90]
              tunnel: [w90] -> w86
              frame #0 {
                # "#CSM External Error Handler Case\nUsually, it's because This CSM register others' \"Error Occurred\" status with \"Error Handler\". If other CSM have any error, the error will be passed here for central handling."
              }
            }
          }
          frame Error {
            # "#CSM Internal Error Handler Case \nIf any error Occurred, \"Error Occurred\" \nstatus update will be broadcasted to system.\nParameter is Error Cluster."
            n30 = call <userlib>:"CSM - Convert Error to Argument.vi"("Error"=w91) -> ("Argument"=w95:string)  [unwired: 4 in]
            n31 = call <vilib>:"Build State String with Arguments__JKI_lib_State_Machine.vi"("Arguments (\"\")"=w95, "State"="Error Occurred" ("Status with Arguments")) -> ("State with Arguments"=w94:string)  [unwired: 4 in]
            n32 = call <userlib>:"CSM - Broadcast Status Change.vi"("Status With Arguments"=w94, "State Queue"=w92) -> ("Remaining States"=w93:string)  [unwired: 13 in]
          }
        }
        "温控-错误输出" <- w75
        n33 = call <vilib>:"Add State(s) to Queue__JKI_lib_State_Machine.vi"("State(s) in Front (\"\")"="// Post Error States", "State(s) in (\"\")"=w81) -> ("States Out"=w80:string)  [unwired: 13 in]
      }
      frame "Critical Error" {
        # "#CSM \"Critical Error\"\nWhen any un-recoverable error occurs, CSM goes into this case."
        # "#CSM Stop in Critical Error\nWhen Critical Error occurs, Stop the loop immediately. Do NOT change this unless you fully understand the impact."
        n34 = call <userlib>:"CSM Critical Error.vi"("error in (no error)"=w98, "Arugments (As Reason)"=w100, "CSM Name"=w99) -> ("error out"=w97:errorcluster)  [unwired: 8 in]
        n35 = call <vilib>:"Add State(s) to Queue__JKI_lib_State_Machine.vi"("State(s) in (\"\")"=w104) -> ("States Out"=w103:string)  [unwired: 14 in]
      }
      frame "Target Timeout Error" {
        # "#CSM \"Target Timeout Error\"\nWhen This CSM could not get the sync-call response in time, This CSM goes into this case."
        n36 = call <userlib>:"CSM Target Timeout Error.vi"("error in (no error)"=w106, "Arguments (As CSM Name)"=w107) -> ("error out"=w105:errorcluster)  [unwired: 9 in]
        n37 = call <vilib>:"Add State(s) to Queue__JKI_lib_State_Machine.vi"("State(s) in (\"\")"=w110) -> ("States Out"=w109:string)  [unwired: 14 in]
      }
      frame "Target Error" {
        # "#CSM \"Target Error\"\nWhen This CSM try to communicate with an un-existed CSM, This CSM goes into this case."
        n38 = call <userlib>:"CSM Target Error.vi"("error in (no error)"=w112, "Arguments (As CSM Name)"=w113) -> ("error out"=w111:errorcluster)  [unwired: 9 in]
        n39 = call <vilib>:"Add State(s) to Queue__JKI_lib_State_Machine.vi"("State(s) in (\"\")"=w116) -> ("States Out"=w115:string)  [unwired: 14 in]
      }
      frame "Async Response", "Response" {
        n40 = Unbundle(w122) -> ("‘State"=w119:string, "’Arguments"=w118:string, "’Error"=w117:errorcluster)
        n41 = case shown="默认" w119 {
          tunnel: [w128] -> w125
          tunnel: w126 -> [w129]
          tunnel: [w131] -> w123
          tunnel: w124 -> [w131]
          tunnel: [w130] -> w127
          tunnel: w117 -> [w130]
          tunnel: w121 -> [_]
          tunnel: w120 -> [_]
          tunnel: w118 -> [_]
          frame 默认 {
            # "#CSM \"Async Response\"\nHandle Async-call Response (\"Async Response\" for ->)"
            # "#CSM \"Response\"\nHandle Sync-call Response (\"Response\" for -@)"
            # "#CSM Response Comments\nAfter Message is executed, CSM goes to this state for receive the response.\n    For Async Message(->), \"Async Response\" is used. This CSM will goes to \"Async Message Posted\" immediately and receive the \"Async Response\" after the callee finishes the message.\n    For Sync Message(@),  This CSM will wait until the message is done and immediately goes to \"Response\""
            n42 = call <vilib>:"Add State(s) to Queue__JKI_lib_State_Machine.vi"("State(s) in (\"\")"=w129) -> ("States Out"=w128:string)  [unwired: 14 in]
          }
        }
      }
      frame "Async Message Posted" {
        # "#CSM \"Async Message Posted\"\nAfter Async Message is posted (-> or ->| ), CSM goes to this state for post-action.\nYou can use Argument - State to tell which Async Message is called."
      }
      frame "Initialize Core Data" {
        # "#CSM \"Initialize Core Data\"\nThis is used to determine panel behavior on exit"
        # "originally closed?"
        # "exe?"
        # "If panel starts closed or is an EXE, then close it when we exit"
        n43 = property class="VI"() -> ("FP.State"=w136:T9)  [unwired: 2 in, 2 out]
        n44 = property class="App"() -> ("App.Kind"=w142:T10)  [unwired: 2 in, 2 out]
        n45 = control-ref of="Current VI Reference"() -> (w137:refnum<vi>)
        n46 = Equal?(x=w136, y=T9."Closed" ("Front Panel Window:State")) -> (x = y?=w134:bool)
        n47 = Equal?(x=w142, y=T10."Run Time System" ("Application:Kind")) -> (x = y?=w140:bool)
        n48 = Or(x=w134, y=w140) -> (x .or. y?=w138:bool)
        n49 = Bundle By Name(cluster=w139, "Core.Current VI Reference"=w137, "Core.Close Panel on Exit?"=w138) -> (w143:T17)
        n50 = call <vilib>:"Add State(s) to Queue__JKI_lib_State_Machine.vi"("State(s) in (\"\")"=w145) -> ("States Out"=w144:string)  [unwired: 14 in]
      }
      frame "Exit" {
        # "#CSM \"Exit\"\nCase for exiting the loop. No errors that occur here will be handled."
        n51 = call <vilib>:"Add State(s) to Queue__JKI_lib_State_Machine.vi"("State(s) in (\"\")"=w149) -> ("States Out"=w148:string)  [unwired: 14 in]
      }
      frame "---------- Data ----------" {
        # "#CSM \"Category Seperator\"\nDo not put any code in this frame."
        n52 = call <vilib>:"Add State(s) to Queue__JKI_lib_State_Machine.vi"("State(s) in (\"\")"=w152) -> ("States Out"=w151:string)  [unwired: 14 in]
      }
      frame "Data: Initialize" {
        w154 = FALSE ("Fast Mode?")
        w157 = T18 {"子程序？"=FALSE, "Fast Mode?"=FALSE, "Auto Range 1?"=FALSE, "Auto Range 2?"=FALSE}  # 其他
        w163 = cluster{"开关 1":bool, "开关 2":bool, "温控是否打开":bool} {"开关 1"=FALSE, "开关 2"=FALSE, "温控是否打开"=FALSE}  # 开关信息
        w164 = T16 {"采集时间"=timestamp(0 s since 1904-01-01), "Data"=[]}  # Time and Data
        w166 = T19 {"过压/过流 1"={"过压保护阈值"=6.0, "过流保护阈值"=3.0}, "过压/过流 2"={"过压保护阈值"=6.0, "过流保护阈值"=3.0}, "保护结果 1"={"过压保护结果"=enum."正常", "过流保护结果"=enum."正常", "过温保护结果"=enum."正常"}, "保护结果 2"={"过压保护结果"=enum."正常", "过流保护结果"=enum."正常", "过温保护结果"=enum."正常"}, "过温 1"={"过温保护开关"=FALSE, "过温保护低阈值"=5.0, "过温保护高阈值"=45.0, "最低设定温度"=5.0, "最高设定温度"=45.0, "温度限速"=0.0}, "过温 2"={"过温保护开关"=FALSE, "过温保护低阈值"=5.0, "过温保护高阈值"=45.0, "最低设定温度"=5.0, "最高设定温度"=45.0, "温度限速"=0.0}}  # 保护
        w165 = cluster{"设备型号":string, "双通道设备？":bool} {"设备型号"="", "双通道设备？"=FALSE}  # 设备信息
        w167 = T20 {"输出设置 1"={"输出模式"=enum."加热模式", "最大输出电压"=5.0}, "输出设置 2"={"输出模式"=enum."加热模式", "最大输出电压"=5.0}, "输出状态 1"={"功率输出"=enum."已关闭", "实际输出电压"=0.0, "实际输出电流"=0.0, "实际输出功率"=0.0}, "输出状态 2"={"功率输出"=enum."已关闭", "实际输出电压"=0.0, "实际输出电流"=0.0, "实际输出功率"=0.0}, "PID 1"={"PID类型"=enum."PID", "P"=0.05, "I"=20.0, "D"=2.0, "PID控制间隔"=0.1, "PID计算方法"=enum."最大正向输出"}, "PID 2"={"PID类型"=enum."PID", "P"=0.05, "I"=20.0, "D"=2.0, "PID控制间隔"=0.1, "PID计算方法"=enum."最大正向输出"}}  # 输出参数
        w168 = T21 {"温控温度 1"=25.0, "实际温度 1"=25.0, "温控温度 2"=25.0, "实际温度 2"=25.0, "打开串口"=FALSE}  # 温控情况
        w159 = T15 {"USB Port"="COM1", "采集间隔(s)"=0.5}  # 基本信息
        w169 = T14 {"Current VI Reference"=refnum, "Close Panel on Exit?"=FALSE}  # Core
        # "#CSM \"Data: Initialize\"\nInitialize the shift-register data, here.\n(data names are defined by what you wire into the bundle function)"
        # "#CSM do not delete - used by framework"
        # "#CSM Expand Bundle to add new data elements to shift register data."
        # "#CSM Data names and types of shift register data are defined by this bundle."
        n53 = call "CSM - Read Cluster Elements From Session.vim"("Section Name (\"\" as Default)"=w162, "Cluster"=w159) -> ("Cluster out"=w160:T15)  [unwired: 6 in, 1 out]
        n54 = local read "Fast Mode"() -> (w153:bool)
        n55 = local read "子程序？"() -> (w156:bool)
        n56 = Select(t=w160, s=TRUE, f=w159) -> (s? t:f=w158:T15)
        n57 = Bundle By Name(cluster=w157, "子程序？"=w156, "Fast Mode?"=w153, "Auto Range 1?"=w154, "Auto Range 2?"=w154) -> (w155:T18)
        n58 = Bundle("Core"=w169, "基本信息"=w158, "温控情况"=w168, "开关信息"=w163, "输出参数"=w167, "保护"=w166, "设备信息"=w165, "Time and Data"=w164, "其他"=w155) -> (w170:T17)  [unwired: 1 in]
        n59 = call <vilib>:"Add State(s) to Queue__JKI_lib_State_Machine.vi"("State(s) in (\"\")"=w172) -> ("States Out"=w171:string)  [unwired: 14 in]
      }
      frame "Data: Update Indicators" {
        w196 = dbl[] [] ("数组")
        w211 = T16 {"采集时间"=timestamp(0 s since 1904-01-01), "Data"=[]}  # Time and Data
        n60 = Unbundle By Name(w183) -> ("输出参数.输出状态 1.功率输出"=w198:enum16{"已关闭", "已打开"}, "输出参数.输出状态 2.功率输出"=w197:enum16{"已关闭", "已打开"}, "设备信息.双通道设备？"=w193:bool)
        n61 = call "CSM - Convert Argument to MassData.vim"("Type"=w211, "MassData Argument"=w205) -> ("Data"=w173:T16)  [unwired: 6 in, 1 out]
        n62 = Index Array(array=w196, index="跟随通道 1") -> (element=w209:dbl)
        n63 = Index Array(array=w196, index="跟随通道 2") -> (element=w208:dbl)
        n64 = Compound Arithmetic op=AND ("复合运算")("是否跟随 2", w193) -> (w195:bool)
        n65 = Unbundle By Name(w173) -> ("Data"=w199:dbl[])
        n66 = case shown="True" "是否跟随 1" {
          tunnel: w209 -> [_ w224]
          tunnel: [_ w223] -> w192
          frame False {
          }
          frame True {
            n67 = Add(x=w224, y="跟随偏移 1") -> (x+y=w225:dbl)
            n68 = property on="温控温度 1" class="DigNum (严格)"("Val(Sgnl)"=w225) -> (error out=w223:errorcluster)  [unwired: 2 in, 1 out]
          }
        }
        n69 = case shown="True" w195 {
          tunnel: w208 -> [_ w230]
          tunnel: w192 -> [_ w227]
          frame False {
          }
          frame True {
            n70 = Add(x=w230, y="跟随偏移 2") -> (x+y=w228:dbl)
            n71 = property on="温控温度 2" class="DigNum (严格)"(error in=w227, "Val(Sgnl)"=w228) -> ()  [unwired: 1 in, 2 out]
          }
        }
        n72 = Index Array(array=w199, index #1=1 ("索引"), index #2=2 ("索引"), index #3=3 ("索引"), index #4=4 ("索引"), index #5=6 ("索引"), index #6=7 ("索引"), index #7=8 ("索引"), index #8=9 ("索引")) -> (element #1=w174:dbl, element #2=w175:dbl, element #3=w176:dbl, element #4=w177:dbl, element #5=w178:dbl, element #6=w179:dbl, element #7=w180:dbl, element #8=w181:dbl)
        "实际温度 1" <- w174
        "实际温度 2" <- w178
        n73 = in-place {
          in-place-border: w181 -> [w222]
          in-place-border: w180 -> [w221]
          in-place-border: w179 -> [w220]
          in-place-border: w178 -> [w219]
          in-place-border: w177 -> [w218]
          in-place-border: w176 -> [w217]
          in-place-border: w175 -> [w216]
          in-place-border: w174 -> [w215]
          in-place-border: w173 -> [w214]
          n74 = in-place-cluster #1(w183) -> ()  [unwired: 9 out]
          n75 = in-place-cluster #1("Time and Data"=w214, "温控情况.实际温度 1"=w215, "输出参数.输出状态 1.实际输出电压"=w216, "输出参数.输出状态 1.实际输出电流"=w217, "输出参数.输出状态 1.实际输出功率"=w218, "温控情况.实际温度 2"=w219, "输出参数.输出状态 2.实际输出电压"=w220, "输出参数.输出状态 2.实际输出电流"=w221, "输出参数.输出状态 2.实际输出功率"=w222) -> (w182:T17)
        }
        n76 = local read "输出状态 1"() -> (w200:T3)
        n77 = Bundle By Name(cluster=w200, "功率输出"=w198, "实际输出电压"=w175, "实际输出电流"=w176) -> (→"输出状态 1":T3)
        n78 = local read "输出状态 2"() -> (w202:T3)
        n79 = Bundle By Name(cluster=w202, "功率输出"=w197, "实际输出电压"=w179, "实际输出电流"=w180) -> (→"输出状态 2":T3)
        n80 = call <vilib>:"Add State(s) to Queue__JKI_lib_State_Machine.vi"("State(s) in Front (\"\")"="UI: Update Graph" ("State(s) in Front (\"\")"), "State(s) in (\"\")"=w212) -> ("States Out"=w213:string)  [unwired: 13 in]
      }
      frame "Data: Cleanup" {
        # "#CSM \"Data: Cleanup\"\nCleanup any data and references, here.\n(this is called automatically, by the Macro: Exit)"
        n81 = Unbundle By Name(w233) -> ("Core.Current VI Reference"=w236:refnum<vi>, "基本信息"=w232:T15)
        n82 = call "CSM - Write Configuration Variable.vim"("Section Name (\"\" as Default)"=w231, "Configuration"=w232) -> ()  [unwired: 6 in, 2 out]
        n83 = Close Reference(reference=w236, error in (no error)=w235) -> (error out=w234:errorcluster)
        n84 = call <vilib>:"Add State(s) to Queue__JKI_lib_State_Machine.vi"("State(s) in (\"\")"=w238) -> ("States Out"=w237:string)  [unwired: 14 in]
      }
      frame "---------- UI ----------" {
        n85 = call <vilib>:"Add State(s) to Queue__JKI_lib_State_Machine.vi"("State(s) in (\"\")"=w240) -> ("States Out"=w239:string)  [unwired: 14 in]
      }
      frame "UI: Initialize" {
        w243 = u8 2 ("Y标尺.标尺调节")
        w256 = FALSE ("结束")
        w258 = TRUE
        w257 = T22."Disabled and Grayed Out" ("禁用")
        w244 = waveform(dbl)[][] [] ("历史数据")
        n86 = property on="TC1" class="WFChart (严格)"("YScale.ScaleFit"=w243) -> ()  [unwired: 2 in, 2 out]
        n87 = property on="TC2" class="WFChart (严格)"("YScale.ScaleFit"=w243) -> ()  [unwired: 2 in, 2 out]
        n88 = property on="TC1" class="WFChart (严格)"("History Data"=w244) -> ()  [unwired: 2 in, 2 out]
        n89 = property on="TC2" class="WFChart (严格)"("History Data"=w244) -> ()  [unwired: 2 in, 2 out]
        n90 = property on="Power 1" class="WFChart (严格)"("History Data"=w244) -> ()  [unwired: 2 in, 2 out]
        n91 = property on="Power 2" class="WFChart (严格)"("History Data"=w244) -> ()  [unwired: 2 in, 2 out]
        n92 = property on="温控开关 总" class="Bool (严格)"("DisabledEnum"=w257) -> ()  [unwired: 2 in, 2 out]
        n93 = property on="温控开关 1" class="Bool (严格)"("DisabledEnum"=w257) -> ()  [unwired: 2 in, 2 out]
        n94 = property on="温控开关 2" class="Bool (严格)"("DisabledEnum"=w257) -> ()  [unwired: 2 in, 2 out]
        n95 = property on="温控温度 1" class="DigNum (严格)"("DisabledEnum"=w257) -> ()  [unwired: 2 in, 2 out]
        n96 = property on="温控温度 2" class="DigNum (严格)"("DisabledEnum"=w257) -> ()  [unwired: 2 in, 2 out]
        n97 = property on="输出设置 1" class="Clust (严格)"("DisabledEnum"=w257) -> ()  [unwired: 2 in, 2 out]
        n98 = property on="输出设置 2" class="Clust (严格)"("DisabledEnum"=w257) -> ()  [unwired: 2 in, 2 out]
        n99 = property on="PID 2" class="Clust (严格)"("DisabledEnum"=w257) -> ()  [unwired: 2 in, 2 out]
        n100 = property on="PID 1" class="Clust (严格)"("DisabledEnum"=w257) -> ()  [unwired: 2 in, 2 out]
        n101 = property on="过温 1" class="Clust (严格)"("DisabledEnum"=w257) -> ()  [unwired: 2 in, 2 out]
        n102 = property on="过温 2" class="Clust (严格)"("DisabledEnum"=w257) -> ()  [unwired: 2 in, 2 out]
        n103 = property on="过压/过流 1" class="Clust (严格)"("DisabledEnum"=w257) -> ()  [unwired: 2 in, 2 out]
        n104 = property on="过压/过流 2" class="Clust (严格)"("DisabledEnum"=w257) -> ()  [unwired: 2 in, 2 out]
        n105 = property on="保护结果 1" class="Clust (严格)"("DisabledEnum"=w257) -> ()  [unwired: 2 in, 2 out]
        n106 = property on="保护结果 2" class="Clust (严格)"("DisabledEnum"=w257) -> ()  [unwired: 2 in, 2 out]
        n107 = property on="温控循环功能" class="Bool (严格)"("DisabledEnum"=w257) -> ()  [unwired: 2 in, 2 out]
        n108 = Unbundle By Name(w245) -> ("温控情况.温控温度 1"=w252:dbl, "温控情况.温控温度 2"=w251:dbl, "温控情况.打开串口"=w255:bool, "开关信息.开关 1"=w254:bool, "开关信息.开关 2"=w253:bool, "基本信息"=w250:T15, "其他.子程序？"=w247:bool)
        n109 = Unbundle By Name(w250) -> ("USB Port"=w249:refnum<visa-resource-name>, "采集间隔(s)"=w248:dbl)
        n110 = local write "温控循环功能"(w256) -> ()
        n111 = local write "Fast Mode"(w256) -> ()
        n112 = local write "温控-错误输出"(errorcluster {"status"=FALSE, "code"=0, "source"=""} ("Error Out")) -> ()
        n113 = local write "通道"(w258) -> ()
        n114 = local write "温度"(w258) -> ()
        n115 = Not(x=w247) -> (.not. x?=w246:bool)
        n116 = local write "温控温度 1"(w252) -> ()
        n117 = local write "温控温度 2"(w251) -> ()
        n118 = local write "打开串口"(w255) -> ()
        n119 = local write "温控开关 1"(w254) -> ()
        n120 = local write "温控开关 2"(w253) -> ()
        n121 = local write "温控串口"(w249) -> ()
        n122 = local write "采集间隔"(w248) -> ()
        n123 = property on="停止" class="Bool"("Visible"=w246) -> ()  [unwired: 2 in, 2 out]
        n124 = call <vilib>:"Add State(s) to Queue__JKI_lib_State_Machine.vi"("State(s) in (\"\")"=w261) -> ("States Out"=w260:string)  [unwired: 14 in]
      }
      frame "UI: Start" {
        w265 = T22."Enabled" ("禁用")
        n125 = Unbundle By Name(w267) -> ("设备信息.双通道设备？"=w266:bool)
        n126 = property on="保护结果 1" class="Clust (严格)"("DisabledEnum"=w265) -> ()  [unwired: 2 in, 2 out]
        n127 = property on="温控循环功能" class="Bool (严格)"("DisabledEnum"=w265) -> ()  [unwired: 2 in, 2 out]
        n128 = property on="温控开关 1" class="Bool (严格)"("DisabledEnum"=w265) -> ()  [unwired: 2 in, 2 out]
        n129 = property on="温控温度 1" class="DigNum (严格)"("DisabledEnum"=w265) -> ()  [unwired: 2 in, 2 out]
        n130 = property on="输出设置 1" class="Clust (严格)"("DisabledEnum"=w265) -> ()  [unwired: 2 in, 2 out]
        n131 = property on="PID 1" class="Clust (严格)"("DisabledEnum"=w265) -> ()  [unwired: 2 in, 2 out]
        n132 = property on="过温 1" class="Clust (严格)"("DisabledEnum"=w265) -> ()  [unwired: 2 in, 2 out]
        n133 = property on="过压/过流 1" class="Clust (严格)"("DisabledEnum"=w265) -> ()  [unwired: 2 in, 2 out]
        n134 = case shown="True" w266 {
          tunnel: w265 -> [_ w270]
          tunnel: w265 -> [_ w269]
          frame False {
          }
          frame True {
            n135 = property on="温控开关 2" class="Bool (严格)"("DisabledEnum"=w270) -> ()  [unwired: 2 in, 2 out]
            n136 = property on="温控温度 2" class="DigNum (严格)"("DisabledEnum"=w270) -> ()  [unwired: 2 in, 2 out]
            n137 = property on="输出设置 2" class="Clust (严格)"("DisabledEnum"=w270) -> ()  [unwired: 2 in, 2 out]
            n138 = property on="PID 2" class="Clust (严格)"("DisabledEnum"=w270) -> ()  [unwired: 2 in, 2 out]
            n139 = property on="过温 2" class="Clust (严格)"("DisabledEnum"=w270) -> ()  [unwired: 2 in, 2 out]
            n140 = property on="过压/过流 2" class="Clust (严格)"("DisabledEnum"=w270) -> ()  [unwired: 2 in, 2 out]
            n141 = property on="保护结果 2" class="Clust (严格)"("DisabledEnum"=w270) -> ()  [unwired: 2 in, 2 out]
            n142 = property on="温控开关 总" class="Bool (严格)"("DisabledEnum"=w269) -> ()  [unwired: 2 in, 2 out]
          }
        }
        n143 = call <vilib>:"Add State(s) to Queue__JKI_lib_State_Machine.vi"("State(s) in (\"\")"=w263) -> ("States Out"=w264:string)  [unwired: 14 in]
      }
      frame "UI: Output1" {
        # "输出模式"
        # "最大输出电压"
        n144 = Unbundle By Name(w286) -> ("基本信息.USB Port"=w285:refnum<visa-resource-name>)
        n145 = call "串口读写 - WK.vi"("错误输入（无错误）"=w284, "写入设备"="TC1:TCADJUSTTEMP?\r" ("写入缓冲区"), "VISA输入"=w285) -> ("错误输出"=w293:errorcluster, "读取设备(n)"=w292:dbl, "VISA输出"=w294:refnum<visa-resource-name>)  [unwired: 5 in, 1 out]
        n146 = local write "温控温度 1"(w292) -> ()
        n147 = call "串口读写 - WK.vi"("错误输入（无错误）"=w293, "写入设备"="TC1:TCSW?\r" ("写入缓冲区"), "VISA输入"=w294) -> ("错误输出"=w275:errorcluster, "读取设备(n)"=w271:dbl, "VISA输出"=w276:refnum<visa-resource-name>)  [unwired: 5 in, 1 out]
        n148 = Not Equal To 0?(x=w271) -> (x != 0?=w289:bool)
        n149 = local read "输出状态 1"() -> (w291:T3)
        n150 = local write "温控开关 1"(w289) -> ()
        n151 = Bundle By Name(cluster=w291, "功率输出"=w271) -> (w290:T3)
        n152 = local write "输出状态 1"(w290) -> ()
        n153 = call "串口读写 - WK.vi"("错误输入（无错误）"=w275, "写入设备"="TC1:TCMAXV?\r" ("写入缓冲区"), "VISA输入"=w276) -> ("错误输出"=w280:errorcluster, "读取设备(n)"=w279:dbl, "VISA输出"=w283:refnum<visa-resource-name>)  [unwired: 5 in, 1 out]
        n154 = call "串口读写 - WK.vi"("错误输入（无错误）"=w280, "写入设备"="TC1:TCMODE?\r" ("写入缓冲区"), "VISA输入"=w283) -> ("错误输出"=w274:errorcluster, "读取设备(n)"=w281:dbl)  [unwired: 5 in, 2 out]
        n155 = local read "输出设置 1"() -> (w282:T4)
        n156 = Bundle By Name(cluster=w282, "输出模式"=w281, "最大输出电压"=w279) -> (w273:T4)
        n157 = Bundle By Name(cluster=w286, "温控情况.温控温度 1"=w292, "开关信息.开关 1"=w289, "输出参数.输出状态 1.功率输出"=w271, "输出参数.输出设置 1"=w273) -> (w272:T17)
        n158 = local write "输出设置 1"(w273) -> ()
        n159 = call <vilib>:"Add State(s) to Queue__JKI_lib_State_Machine.vi"("State(s) in (\"\")"=w295) -> ("States Out"=w296:string)  [unwired: 14 in]
      }
      frame "UI: Output2" {
        n160 = Unbundle By Name(w314) -> ("基本信息.USB Port"=w315:refnum<visa-resource-name>)
        n161 = call "串口读写 - WK.vi"("错误输入（无错误）"=w299, "写入设备"="TC2:TCADJUSTTEMP?\r" ("写入缓冲区"), "VISA输入"=w315) -> ("错误输出"=w318:errorcluster, "读取设备(n)"=w300:dbl, "VISA输出"=w319:refnum<visa-resource-name>)  [unwired: 5 in, 1 out]
        n162 = local write "温控温度 2"(w300) -> ()
        n163 = call "串口读写 - WK.vi"("错误输入（无错误）"=w318, "写入设备"="TC2:TCSW?\r" ("写入缓冲区"), "VISA输入"=w319) -> ("错误输出"=w304:errorcluster, "读取设备(n)"=w297:dbl, "VISA输出"=w305:refnum<visa-resource-name>)  [unwired: 5 in, 1 out]
        n164 = Not Equal To 0?(x=w297) -> (x != 0?=w301:bool)
        n165 = local read "输出状态 2"() -> (w320:T3)
        n166 = local write "温控开关 2"(w301) -> ()
        n167 = Bundle By Name(cluster=w320, "功率输出"=w297) -> (w302:T3)
        n168 = local write "输出状态 2"(w302) -> ()
        n169 = call "串口读写 - WK.vi"("错误输入（无错误）"=w304, "写入设备"="TC2:TCMAXV?\r" ("写入缓冲区"), "VISA输入"=w305) -> ("错误输出"=w311:errorcluster, "读取设备(n)"=w312:dbl, "VISA输出"=w308:refnum<visa-resource-name>)  [unwired: 5 in, 1 out]
        n170 = local read "输出设置 2"() -> (w310:T4)
        n171 = call "串口读写 - WK.vi"("错误输入（无错误）"=w311, "写入设备"="TC2:TCMODE?\r" ("写入缓冲区"), "VISA输入"=w308) -> ("错误输出"=w298:errorcluster, "读取设备(n)"=w309:dbl)  [unwired: 5 in, 2 out]
        n172 = Bundle By Name(cluster=w310, "输出模式"=w309, "最大输出电压"=w312) -> (w303:T4)
        n173 = local write "输出设置 2"(w303) -> ()
        n174 = Bundle By Name(cluster=w314, "温控情况.温控温度 2"=w300, "开关信息.开关 2"=w301, "输出参数.输出状态 2.功率输出"=w297, "输出参数.输出设置 2"=w303) -> (w313:T17)
        n175 = call <vilib>:"Add State(s) to Queue__JKI_lib_State_Machine.vi"("State(s) in (\"\")"=w321) -> ("States Out"=w322:string)  [unwired: 14 in]
      }
      frame "UI: PID1" {
        # "控制间隔"
        # "D值"
        # "I值"
        # "P值"
        # "PID类型"
        n176 = Unbundle By Name(w326) -> ("基本信息.USB Port"=w328:refnum<visa-resource-name>)
        n177 = call "串口读写 - WK.vi"("错误输入（无错误）"=w324, "写入设备"="TC1:TCPIDTYPE?\r" ("写入缓冲区"), "VISA输入"=w328) -> ("错误输出"=w347:errorcluster, "读取设备(n)"=w339:dbl, "VISA输出"=w351:refnum<visa-resource-name>)  [unwired: 5 in, 1 out]
        n178 = call "串口读写 - WK.vi"("错误输入（无错误）"=w347, "写入设备"="TC1:TCP?\r" ("写入缓冲区"), "VISA输入"=w351) -> ("错误输出"=w346:errorcluster, "读取设备(n)"=w340:dbl, "VISA输出"=w350:refnum<visa-resource-name>)  [unwired: 5 in, 1 out]
        n179 = call "串口读写 - WK.vi"("错误输入（无错误）"=w346, "写入设备"="TC1:TCTI?\r" ("写入缓冲区"), "VISA输入"=w350) -> ("错误输出"=w345:errorcluster, "读取设备(n)"=w341:dbl, "VISA输出"=w349:refnum<visa-resource-name>)  [unwired: 5 in, 1 out]
        n180 = call "串口读写 - WK.vi"("错误输入（无错误）"=w345, "写入设备"="TC1:TCTD?\r" ("写入缓冲区"), "VISA输入"=w349) -> ("错误输出"=w344:errorcluster, "读取设备(n)"=w342:dbl, "VISA输出"=w348:refnum<visa-resource-name>)  [unwired: 5 in, 1 out]
        n181 = call "串口读写 - WK.vi"("错误输入（无错误）"=w344, "写入设备"="TC1:TCCTRLINTERVAL?\r" ("写入缓冲区"), "VISA输入"=w348) -> ("错误输出"=w336:errorcluster, "读取设备(n)"=w338:dbl, "VISA输出"=w337:refnum<visa-resource-name>)  [unwired: 5 in, 1 out]
        n182 = call "串口读写 - WK.vi"("错误输入（无错误）"=w336, "写入设备"="TC1:TCPIDCAL?\r" ("写入缓冲区"), "VISA输入"=w337) -> ("错误输出"=w323:errorcluster, "读取设备(n)"=w335:dbl)  [unwired: 5 in, 2 out]
        n183 = local read "PID 1"() -> (w343:T5)
        n184 = Bundle By Name(cluster=w343, "PID类型"=w339, "P"=w340, "I"=w341, "D"=w342, "PID控制间隔"=w338, "PID计算方法"=w335) -> (w327:T5)
        n185 = local write "PID 1"(w327) -> ()
        n186 = Bundle By Name(cluster=w326, "输出参数.PID 1"=w327) -> (w325:T17)
        n187 = call <vilib>:"Add State(s) to Queue__JKI_lib_State_Machine.vi"("State(s) in (\"\")"=w352) -> ("States Out"=w353:string)  [unwired: 14 in]
      }
      frame "UI: PID2" {
        # "控制间隔"
        # "D值"
        # "I值"
        # "P值"
        # "PID类型"
        n188 = Unbundle By Name(w357) -> ("基本信息.USB Port"=w356:refnum<visa-resource-name>)
        n189 = call "串口读写 - WK.vi"("错误输入（无错误）"=w355, "写入设备"="TC2:TCPIDTYPE?\r" ("写入缓冲区"), "VISA输入"=w356) -> ("错误输出"=w369:errorcluster, "读取设备(n)"=w374:dbl, "VISA输出"=w365:refnum<visa-resource-name>)  [unwired: 5 in, 1 out]
        n190 = call "串口读写 - WK.vi"("错误输入（无错误）"=w369, "写入设备"="TC2:TCP?\r" ("写入缓冲区"), "VISA输入"=w365) -> ("错误输出"=w370:errorcluster, "读取设备(n)"=w375:dbl, "VISA输出"=w366:refnum<visa-resource-name>)  [unwired: 5 in, 1 out]
        n191 = call "串口读写 - WK.vi"("错误输入（无错误）"=w370, "写入设备"="TC2:TCTI?\r" ("写入缓冲区"), "VISA输入"=w366) -> ("错误输出"=w371:errorcluster, "读取设备(n)"=w376:dbl, "VISA输出"=w367:refnum<visa-resource-name>)  [unwired: 5 in, 1 out]
        n192 = call "串口读写 - WK.vi"("错误输入（无错误）"=w371, "写入设备"="TC2:TCTD?\r" ("写入缓冲区"), "VISA输入"=w367) -> ("错误输出"=w372:errorcluster, "读取设备(n)"=w377:dbl, "VISA输出"=w368:refnum<visa-resource-name>)  [unwired: 5 in, 1 out]
        n193 = call "串口读写 - WK.vi"("错误输入（无错误）"=w372, "写入设备"="TC2:TCCTRLINTERVAL?\r" ("写入缓冲区"), "VISA输入"=w368) -> ("错误输出"=w380:errorcluster, "读取设备(n)"=w378:dbl, "VISA输出"=w379:refnum<visa-resource-name>)  [unwired: 5 in, 1 out]
        n194 = call "串口读写 - WK.vi"("错误输入（无错误）"=w380, "写入设备"="TC2:TCPIDCAL?\r" ("写入缓冲区"), "VISA输入"=w379) -> ("错误输出"=w354:errorcluster, "读取设备(n)"=w381:dbl)  [unwired: 5 in, 2 out]
        n195 = local read "PID 2"() -> (w373:T5)
        n196 = Bundle By Name(cluster=w373, "PID类型"=w374, "P"=w375, "I"=w376, "D"=w377, "PID控制间隔"=w378, "PID计算方法"=w381) -> (w358:T5)
        n197 = local write "PID 2"(w358) -> ()
        n198 = call <vilib>:"Add State(s) to Queue__JKI_lib_State_Machine.vi"("State(s) in (\"\")"=w383) -> ("States Out"=w384:string)  [unwired: 14 in]
        n199 = Bundle By Name(cluster=w357, "输出参数.PID 2"=w358) -> (w382:T17)
      }
      frame "UI: Protect1" {
        # "温度限速"
        # "最高设定温度"
        # "最低设定温度"
        # "过温保护高阈值"
        # "过温保护低阈值"
        # "过温保护开关"
        # "过温保护结果"
        # "过流保护结果"
        # "过压保护结果"
        # "过流保护"
        # "过压保护"
        n200 = Unbundle By Name(w417) -> ("设备信息.设备型号"=w433:string, "基本信息.USB Port"=w439:refnum<visa-resource-name>)
        n201 = Equal?(x="TCM1040\r" ("y"), y=w433) -> (x = y?=w418:bool)
        n202 = call "串口读写 - WK.vi"("错误输入（无错误）"=w387, "写入设备"="TC1:TCADJUSTOVPV?\r" ("写入缓冲区"), "VISA输入"=w439) -> ("错误输出"=w437:errorcluster, "读取设备(n)"=w435:dbl, "VISA输出"=w438:refnum<visa-resource-name>)  [unwired: 5 in, 1 out]
        n203 = case shown="False" w418 {
          tunnel: w438 -> [w455 w458]
          tunnel: [w454 w458] -> w420
          tunnel: [w453 w459] -> w419
          tunnel: w437 -> [w452 w459]
          tunnel: [w451 2.0 ("读取设备(n)")] -> w434
          frame False {
            n204 = call "串口读写 - WK.vi"("错误输入（无错误）"=w452, "写入设备"="TC1:TCADJUSTOCPC?\r" ("写入缓冲区"), "VISA输入"=w455) -> ("错误输出"=w453:errorcluster, "读取设备(n)"=w451:dbl, "VISA输出"=w454:refnum<visa-resource-name>)  [unwired: 5 in, 1 out]
          }
          frame True {
          }
        }
        n205 = local read "过压/过流 1"() -> (w436:cluster{"过压保护阈值":dbl, "过流保护阈值":dbl})
        n206 = Bundle By Name(cluster=w436, "过压保护阈值"=w435, "过流保护阈值"=w434) -> (w416:cluster{"过压保护阈值":dbl, "过流保护阈值":dbl})
        n207 = local write "过压/过流 1"(w416) -> ()
        n208 = call "串口读写 - WK.vi"("错误输入（无错误）"=w419, "写入设备"="TC1:TCOVEF?\r" ("写入缓冲区"), "VISA输入"=w420) -> ("错误输出"=w428:errorcluster, "读取设备(n)"=w425:dbl, "VISA输出"=w430:refnum<visa-resource-name>)  [unwired: 5 in, 1 out]
        n209 = case shown="False" w418 {
          tunnel: w430 -> [w446 w450]
          tunnel: [w445 w450] -> w429
          tunnel: w428 -> [w444 w449]
          tunnel: [w443 w449] -> w427
          tunnel: [w442 1.0 ("读取设备(n)")] -> w424
          frame False {
            n210 = call "串口读写 - WK.vi"("错误输入（无错误）"=w444, "写入设备"="TC1:TCOCEF?\r" ("写入缓冲区"), "VISA输入"=w446) -> ("错误输出"=w443:errorcluster, "读取设备(n)"=w442:dbl, "VISA输出"=w445:refnum<visa-resource-name>)  [unwired: 5 in, 1 out]
          }
          frame True {
          }
        }
        n211 = call "串口读写 - WK.vi"("错误输入（无错误）"=w427, "写入设备"="TC1:TCOTEF?\r" ("写入缓冲区"), "VISA输入"=w429) -> ("错误输出"=w389:errorcluster, "读取设备(n)"=w423:dbl, "VISA输出"=w390:refnum<visa-resource-name>)  [unwired: 5 in, 1 out]
        n212 = call "串口读写 - WK.vi"("错误输入（无错误）"=w389, "写入设备"="TC1:TCOTPE?\r" ("写入缓冲区"), "VISA输入"=w390) -> ("错误输出"=w410:errorcluster, "读取设备(n)"=w405:dbl, "VISA输出"=w414:refnum<visa-resource-name>)  [unwired: 5 in, 1 out]
        n213 = Not Equal To 0?(x=w405) -> (x != 0?=w404:bool)
        n214 = call "串口读写 - WK.vi"("错误输入（无错误）"=w410, "写入设备"="TC1:TCOTPLT?\r" ("写入缓冲区"), "VISA输入"=w414) -> ("错误输出"=w409:errorcluster, "读取设备(n)"=w403:dbl, "VISA输出"=w413:refnum<visa-resource-name>)  [unwired: 5 in, 1 out]
        n215 = call "串口读写 - WK.vi"("错误输入（无错误）"=w409, "写入设备"="TC1:TCOTPHT?\r" ("写入缓冲区"), "VISA输入"=w413) -> ("错误输出"=w408:errorcluster, "读取设备(n)"=w402:dbl, "VISA输出"=w412:refnum<visa-resource-name>)  [unwired: 5 in, 1 out]
        n216 = call "串口读写 - WK.vi"("错误输入（无错误）"=w408, "写入设备"="TC1:TCMINSETTEMP?\r" ("写入缓冲区"), "VISA输入"=w412) -> ("错误输出"=w407:errorcluster, "读取设备(n)"=w401:dbl, "VISA输出"=w411:refnum<visa-resource-name>)  [unwired: 5 in, 1 out]
        n217 = call "串口读写 - WK.vi"("错误输入（无错误）"=w407, "写入设备"="TC1:TCMAXSETTEMP?\r" ("写入缓冲区"), "VISA输入"=w411) -> ("错误输出"=w398:errorcluster, "读取设备(n)"=w400:dbl, "VISA输出"=w399:refnum<visa-resource-name>)  [unwired: 5 in, 1 out]
        n218 = call "串口读写 - WK.vi"("错误输入（无错误）"=w398, "写入设备"="TC1:TCRAMPSPEED?\r" ("写入缓冲区"), "VISA输入"=w399) -> ("错误输出"=w386:errorcluster, "读取设备(n)"=w397:dbl)  [unwired: 5 in, 2 out]
        n219 = local read "过温 1"() -> (w406:T6)
        n220 = local read "保护结果 1"() -> (w426:T7)
        n221 = Bundle By Name(cluster=w406, "过温保护开关"=w404, "过温保护低阈值"=w403, "过温保护高阈值"=w402, "最低设定温度"=w401, "最高设定温度"=w400, "温度限速"=w397) -> (w388:T6)
        n222 = Bundle By Name(cluster=w426, "过压保护结果"=w425, "过流保护结果"=w424, "过温保护结果"=w423) -> (w385:T7)
        "保护结果 1" <- w385
        n223 = local write "过温 1"(w388) -> ()
        n224 = call <vilib>:"Add State(s) to Queue__JKI_lib_State_Machine.vi"("State(s) in (\"\")"=w440) -> ("States Out"=w441:string)  [unwired: 14 in]
        n225 = Bundle By Name(cluster=w417, "保护.过压/过流 1"=w416, "保护.保护结果 1"=w385, "保护.过温 1"=w388) -> (w415:T17)
      }
      frame "UI: Protect2" {
        # "温度限速"
        # "最高设定温度"
        # "最低设定温度"
        # "过温保护高阈值"
        # "过温保护低阈值"
        # "过温保护开关"
        # "过流保护"
        # "过压保护"
        # "过温保护结果"
        # "过流保护结果"
        # "过压保护结果"
        n226 = Unbundle By Name(w495) -> ("基本信息.USB Port"=w493:refnum<visa-resource-name>)
        n227 = call "串口读写 - WK.vi"("错误输入（无错误）"=w462, "写入设备"="TC2:TCADJUSTOVPV?\r" ("写入缓冲区"), "VISA输入"=w493) -> ("错误输出"=w499:errorcluster, "读取设备(n)"=w500:dbl, "VISA输出"=w498:refnum<visa-resource-name>)  [unwired: 5 in, 1 out]
        n228 = call "串口读写 - WK.vi"("错误输入（无错误）"=w499, "写入设备"="TC2:TCADJUSTOCPC?\r" ("写入缓冲区"), "VISA输入"=w498) -> ("错误输出"=w491:errorcluster, "读取设备(n)"=w501:dbl, "VISA输出"=w492:refnum<visa-resource-name>)  [unwired: 5 in, 1 out]
        n229 = local read "过压/过流 2"() -> (w502:cluster{"过压保护阈值":dbl, "过流保护阈值":dbl})
        n230 = Bundle By Name(cluster=w502, "过压保护阈值"=w500, "过流保护阈值"=w501) -> (w490:cluster{"过压保护阈值":dbl, "过流保护阈值":dbl})
        n231 = local write "过压/过流 2"(w490) -> ()
        n232 = call "串口读写 - WK.vi"("错误输入（无错误）"=w491, "写入设备"="TC2:TCOVEF?\r" ("写入缓冲区"), "VISA输入"=w492) -> ("错误输出"=w511:errorcluster, "读取设备(n)"=w509:dbl, "VISA输出"=w513:refnum<visa-resource-name>)  [unwired: 5 in, 1 out]
        n233 = call "串口读写 - WK.vi"("错误输入（无错误）"=w511, "写入设备"="TC2:TCOCEF?\r" ("写入缓冲区"), "VISA输入"=w513) -> ("错误输出"=w510:errorcluster, "读取设备(n)"=w508:dbl, "VISA输出"=w512:refnum<visa-resource-name>)  [unwired: 5 in, 1 out]
        n234 = call "串口读写 - WK.vi"("错误输入（无错误）"=w510, "写入设备"="TC2:TCOTEF?\r" ("写入缓冲区"), "VISA输入"=w512) -> ("错误输出"=w464:errorcluster, "读取设备(n)"=w507:dbl, "VISA输出"=w465:refnum<visa-resource-name>)  [unwired: 5 in, 1 out]
        n235 = call "串口读写 - WK.vi"("错误输入（无错误）"=w464, "写入设备"="TC2:TCOTPE?\r" ("写入缓冲区"), "VISA输入"=w465) -> ("错误输出"=w476:errorcluster, "读取设备(n)"=w480:dbl, "VISA输出"=w472:refnum<visa-resource-name>)  [unwired: 5 in, 1 out]
        n236 = Not Equal To 0?(x=w480) -> (x != 0?=w481:bool)
        n237 = call "串口读写 - WK.vi"("错误输入（无错误）"=w476, "写入设备"="TC2:TCOTPLT?\r" ("写入缓冲区"), "VISA输入"=w472) -> ("错误输出"=w477:errorcluster, "读取设备(n)"=w482:dbl, "VISA输出"=w473:refnum<visa-resource-name>)  [unwired: 5 in, 1 out]
        n238 = call "串口读写 - WK.vi"("错误输入（无错误）"=w477, "写入设备"="TC2:TCOTPHT?\r" ("写入缓冲区"), "VISA输入"=w473) -> ("错误输出"=w478:errorcluster, "读取设备(n)"=w483:dbl, "VISA输出"=w474:refnum<visa-resource-name>)  [unwired: 5 in, 1 out]
        n239 = call "串口读写 - WK.vi"("错误输入（无错误）"=w478, "写入设备"="TC2:TCMINSETTEMP?\r" ("写入缓冲区"), "VISA输入"=w474) -> ("错误输出"=w479:errorcluster, "读取设备(n)"=w484:dbl, "VISA输出"=w475:refnum<visa-resource-name>)  [unwired: 5 in, 1 out]
        n240 = call "串口读写 - WK.vi"("错误输入（无错误）"=w479, "写入设备"="TC2:TCMAXSETTEMP?\r" ("写入缓冲区"), "VISA输入"=w475) -> ("错误输出"=w487:errorcluster, "读取设备(n)"=w485:dbl, "VISA输出"=w486:refnum<visa-resource-name>)  [unwired: 5 in, 1 out]
        n241 = call "串口读写 - WK.vi"("错误输入（无错误）"=w487, "写入设备"="TC2:TCRAMPSPEED?\r" ("写入缓冲区"), "VISA输入"=w486) -> ("错误输出"=w461:errorcluster, "读取设备(n)"=w488:dbl)  [unwired: 5 in, 2 out]
        n242 = local read "保护结果 2"() -> (w506:T7)
        n243 = Bundle By Name(cluster=w506, "过压保护结果"=w509, "过流保护结果"=w508, "过温保护结果"=w507) -> (w460:T7)
        "保护结果 2" <- w460
        n244 = local read "过温 2"() -> (w489:T6)
        n245 = Bundle By Name(cluster=w489, "过温保护开关"=w481, "过温保护低阈值"=w482, "过温保护高阈值"=w483, "最低设定温度"=w484, "最高设定温度"=w485, "温度限速"=w488) -> (w463:T6)
        n246 = local write "过温 2"(w463) -> ()
        n247 = call <vilib>:"Add State(s) to Queue__JKI_lib_State_Machine.vi"("State(s) in (\"\")"=w514) -> ("States Out"=w515:string)  [unwired: 14 in]
        n248 = Bundle By Name(cluster=w495, "保护.过压/过流 2"=w490, "保护.保护结果 2"=w460, "保护.过温 2"=w463) -> (w494:T17)
      }
      frame "UI: Update Graph" {
        n249 = Unbundle By Name(w516) -> ("温控情况.温控温度 1"=w538:dbl, "温控情况.实际温度 1"=w539:dbl, "温控情况.温控温度 2"=w537:dbl, "温控情况.实际温度 2"=w536:dbl, "Time and Data.采集时间"=w529:timestamp, "输出参数.输出状态 1.实际输出电压"=w525:dbl, "输出参数.输出状态 2.实际输出电压"=w524:dbl, "基本信息.采集间隔(s)"=w528:dbl, "开关信息.开关 1"=w527:bool, "开关信息.开关 2"=w526:bool)  [unwired: 2 out]
        n250 = Multiply(x=w524, y=w524) -> (x*y=w530:dbl)
        n251 = Multiply(x=w525, y=w525) -> (x*y=w531:dbl)
        n252 = local write "温控开关 1"(w527) -> ()
        n253 = local write "温控开关 2"(w526) -> ()
        n254 = Build Array(w538) -> (w544:dbl[])
        n255 = Build Array(w531) -> (w532:dbl[])
        n256 = Build Array(w537) -> (w543:dbl[])
        n257 = Build Array(w530) -> (w533:dbl[])
        n258 = Build Array(w539) -> (w541:dbl[])
        n259 = Build Array(w536) -> (w542:dbl[])
        n260 = Bundle By Name("Y"=w532, "t0"=w529, "dt"=w528) -> (w523:waveform(dbl))  [unwired: 1 in]
        n261 = Bundle By Name("Y"=w544, "t0"=w529, "dt"=w528) -> (w519:waveform(dbl))  [unwired: 1 in]
        n262 = Bundle By Name("Y"=w543, "t0"=w529, "dt"=w528) -> (w517:waveform(dbl))  [unwired: 1 in]
        n263 = Bundle By Name("Y"=w533, "t0"=w529, "dt"=w528) -> (w518:waveform(dbl))  [unwired: 1 in]
        n264 = Bundle By Name("Y"=w541, "t0"=w529, "dt"=w528) -> (w521:waveform(dbl))  [unwired: 1 in]
        n265 = Bundle By Name("Y"=w542, "t0"=w529, "dt"=w528) -> (w540:waveform(dbl))  [unwired: 1 in]
        n266 = Build Array(w518, w517) -> (→"Power 2":waveform(dbl)[])
        n267 = Build Array(w517, w540) -> (→"TC2":waveform(dbl)[])
        n268 = Build Array(w523, w519) -> (→"Power 1":waveform(dbl)[])
        n269 = Build Array(w519, w521) -> (→"TC1":waveform(dbl)[])
        n270 = call <vilib>:"Add State(s) to Queue__JKI_lib_State_Machine.vi"("State(s) in (\"\")"=w546) -> ("States Out"=w545:string)  [unwired: 14 in]
      }
      frame "UI: Auto Range Change" {
        n271 = property on="TC1" class="WFChart (严格)"() -> ("YScale.Maximum"=w548:dbl)  [unwired: 2 in, 2 out]
        n272 = property on="TC1" class="WFChart (严格)"() -> ("YScale.Minimum"=w549:dbl)  [unwired: 2 in, 2 out]
        n273 = property on="TC2" class="WFChart (严格)"() -> ("YScale.Maximum"=w550:dbl)  [unwired: 2 in, 2 out]
        n274 = property on="TC2" class="WFChart (严格)"() -> ("YScale.Minimum"=w551:dbl)  [unwired: 2 in, 2 out]
        n275 = local write "上限 1"(w548) -> ()
        n276 = local write "下限 1"(w549) -> ()
        n277 = local write "上限 2"(w550) -> ()
        n278 = local write "下限 2"(w551) -> ()
      }
      frame "UI: Gragh Range" {
        n279 = property on="TC1" class="WFChart (严格)"() -> ("YScale.ScaleFit"=w556:u8)  [unwired: 2 in, 2 out]
        n280 = property on="TC2" class="WFChart (严格)"() -> ("YScale.ScaleFit"=w555:u8)  [unwired: 2 in, 2 out]
        n281 = case shown="0" w556 {
          frame 2, Default {
          }
          frame 0 {
            n282 = property on="TC1" class="WFChart (严格)"("YScale.Maximum"="上限 1") -> ()  [unwired: 2 in, 2 out]
            n283 = property on="TC1" class="WFChart (严格)"("YScale.Minimum"="下限 1") -> ()  [unwired: 2 in, 2 out]
          }
        }
        n284 = case shown="0" w555 {
          frame 0 {
            n285 = property on="TC2" class="WFChart (严格)"("YScale.Maximum"="上限 2") -> ()  [unwired: 2 in, 2 out]
            n286 = property on="TC2" class="WFChart (严格)"("YScale.Minimum"="下限 2") -> ()  [unwired: 2 in, 2 out]
          }
          frame 2, Default {
          }
        }
        n287 = call <vilib>:"Add State(s) to Queue__jki_lib_state_machine.vi"("State(s) in (\"\")"=w558) -> ("States Out"=w559:string)  [unwired: 14 in]
      }
      frame "---------- Macro ----------" {
        # "#CSM \"Category Seperator\"\nDo not put any code in this frame."
        n288 = call <vilib>:"Add State(s) to Queue__JKI_lib_State_Machine.vi"("State(s) in (\"\")"=w567) -> ("States Out"=w566:string)  [unwired: 14 in]
      }
      frame "Macro: Initialize" {
        w570 = "Data: Initialize\nInitialize Core Data\nData: Update Indicators\n\nUI: Initialize\n\n//Permanent registrations\nAcquired Data@Acquisition - <1> >> Data: Update Indicators -><register>\nAcquired Data@Acquisition - <1> >> API: Log@Logging - <1> -><register>\n\n//Error registrations\nError Occurred@Acquisition - <1> >> Error Handler -><register>\nError Occurred@Logging - <1> >> Error Handler -><register>\n\n//Dynamic registrations\n// 订阅/取消订阅\n//Status@SourceModule >> API@TargetModule -><register as interrupt>\n//UrgentEvent @SourceModule >> API@TargetModule -><register as status>"  # Data: Initialize Initialize Core Data Data: Update Indicators  UI: Initialize  //Permanent registrations Acquired Data@Acquisition - <1> >> Data: Update Indicators -><register> Acquired Data@Acquisition - <1> >> API: Log@Logging - <1> -><register>  //Error registrations Error Occurred@Acquisition - <1> >> Error Handler -><register> Error Occurred@Logging - <1> >> Error Handler -><register>  //Dynamic registrations // 订阅/取消订阅 //Status@SourceModule >> API@TargetModule -><register as interrupt> //UrgentEvent @SourceModule >> API@TargetModule -><register as status>
        # "#CSM \"Macro: Initialize\"\nInitialization Macro (This is called once, when the VI starts)"
        n289 = call-poly <userlib>:"Build Message with Arguments++.vi"("States With Replace Token"=w570, "<1>"=w569) -> ("States"=w568:string)  [unwired: 13 in]
        n290 = call <vilib>:"Add State(s) to Queue__JKI_lib_State_Machine.vi"("State(s) in Front (\"\")"=w568, "State(s) in (\"\")"=w573) -> ("States Out"=w572:string)  [unwired: 13 in]
      }
      frame "Macro: Start" {
        n291 = Unbundle By Name(T12 {"波特率"=57600, "数据位"=8, "校验"=enum."None", "停止位"=10, "流控制"=0} ("串口设置")) -> ("波特率"=w615:u32, "数据位"=w614:u16, "校验"=w613:enum16{"None", "Odd", "Even", "Mark", "Space"}, "停止位"=w616:u16, "流控制"=w617:u16)
        n292 = call-poly "VISA Configure Serial Port"("VISA resource name"="温控串口", "baud rate (9600)"=w615, "data bits (8)"=w614, "parity (0:none)"=w613, "stop bits (10: 1 bit)"=w616, "flow control (0:none)"=w617) -> ("VISA resource name out"=w611:refnum<visa-resource-name>, "error out"=w609:errorcluster)  [unwired: 3 in, 5 out]
        n293 = Concatenate Strings("MEMORY:MEMWP=" ("写入缓冲区"), "0" ("字符串"), "\r" ("写入缓冲区")) -> (w612:string)
        n294 = local read "采集间隔"() -> (w583:dbl)
        n295 = call "串口读写 - WK.vi"("错误输入（无错误）"=w609, "写入设备"=w612, "VISA输入"=w611) -> ("错误输出"=w608:errorcluster, "VISA输出"=w610:refnum<visa-resource-name>)  [unwired: 5 in, 2 out]
        n296 = call "串口读写 - WK.vi"("错误输入（无错误）"=w608, "写入设备"="SYSTEM:SYSMODEL?\r" ("写入缓冲区"), "VISA输入"=w610) -> ("读取设备"=w596:string)  [unwired: 5 in, 3 out]
        "温控器设备型号" <- w596
        n297 = Not Equal?(x=w596, y="TCM1031\r") -> (x != y?=w607:bool)
        n298 = Not Equal?(x=w596, y="TCM1040\r") -> (x != y?=w606:bool)
        n299 = Compound Arithmetic op=AND(w607, w606) -> (w587:bool)
        n300 = Bundle By Name(cluster=w598, "基本信息.USB Port"="温控串口", "基本信息.采集间隔(s)"=w583, "设备信息.设备型号"=w596, "设备信息.双通道设备？"=w587, "温控情况.打开串口"=TRUE) -> (w592:T17)
        n301 = Unbundle By Name(w592) -> ("基本信息"=w581:T15, "设备信息"=w591:cluster{"设备型号":string, "双通道设备？":bool}, "开关信息"=w585:cluster{"开关 1":bool, "开关 2":bool, "温控是否打开":bool}, "温控情况.温控温度 1"=w580:dbl, "温控情况.温控温度 2"=w579:dbl)
        n302 = Bundle("温控温度 1"=w580, "温控温度 2"=w579) -> (w578:cluster{"温控温度 1":dbl, "温控温度 2":dbl})  [unwired: 1 in]
        n303 = Bundle(cluster=T11 {"基本信息"={"USB Port"="", "采集间隔(s)"=0.0}, "设备信息"={"设备型号"="", "双通道设备？"=FALSE}, "开关"={"开关 1"=FALSE, "开关 2"=FALSE, "Fast Mode"=FALSE}, "Control Temp"={"Control Temp 1"=0.0, "Control Temp 2"=0.0}} ("Device Info"), "基本信息"=w581, "设备信息"=w591, "开关"=w585, "Control Temp"=w578) -> (w590:T11)
        n304 = Select(t="UI: Output2\nUI: PID2\nUI: Protect2" ("State"), s=w587, f="") -> (s? t:f=w576:string)
        n305 = call "Convert Data To API String Arguments.vim"("Data"=w590) -> ("API String"=w594:string)  [unwired: 7 in, 1 out]
        n306 = call-poly <userlib>:"Build Message with Arguments++.vi"("States With Replace Token"="API: Start >> <param> -@ Acquisition - <1>\nAPI: Start  -@ Logging - <1>\n\nUI: Start\n" ("State"), "<param>"=w594, "<1>"=w593) -> ("States"=w575:string)  [unwired: 12 in]
        n307 = call <vilib>:"Add State(s) to Queue__JKI_lib_State_Machine.vi"("State(s) in Front (\"\")"=w575, "State(s) in (\"\")"="UI: Output1\nUI: PID1\nUI: Protect1" ("State"), "State(s) at Back (\"\")"=w576) -> ("States Out"=w574:string)  [unwired: 12 in]
        n308 = call <vilib>:"Add State(s) to Queue__JKI_lib_State_Machine.vi"("State(s) in Front (\"\")"=w574, "State(s) in (\"\")"=w619) -> ("States Out"=w618:string)  [unwired: 13 in]
      }
      frame "Macro: Close" {
        w627 = FALSE ("打开串口")
        n309 = Unbundle By Name(w620) -> ("温控情况.打开串口"=w624:bool, "开关信息.开关 1"=w621:bool, "开关信息.开关 2"=w622:bool, "设备信息.双通道设备？"=w625:bool, "基本信息.USB Port"=w626:refnum<visa-resource-name>)
        n310 = And(x=w622, y=w625) -> (x .and. y?=w623:bool)
        n311 = case shown="True" w624 {
          tunnel: w626 -> [_ w637]
          tunnel: w623 -> [_ w645]
          tunnel: w630 -> [w633 w634]
          tunnel: [w633 w640] -> w629
          tunnel: w621 -> [_ w639]
          frame False {
          }
          frame True {
            n312 = property class="Instr"(reference=w637, error in=w634, "General Settings:Timeout Value"=u32 1000) -> (reference out=w636:refnum<visa-resource-name>, error out=w635:errorcluster)
            n313 = case shown="True" w639 {
              tunnel: w636 -> [w647 w652]
              tunnel: [w647 w650] -> w644
              tunnel: [w646 w649] -> w641
              tunnel: w635 -> [w646 w648]
              frame False {
              }
              frame True {
                n314 = call "串口读写 - WK.vi"("错误输入（无错误）"=w648, "写入设备"="TC1:TCSW=0\r" ("写入缓冲区"), "VISA输入"=w652) -> ("错误输出"=w649:errorcluster, "VISA输出"=w650:refnum<visa-resource-name>)  [unwired: 5 in, 2 out]
              }
            }
            n315 = case shown="True" w645 {
              tunnel: w644 -> [w654 w658]
              tunnel: w641 -> [w653 w657]
              tunnel: [w653 w656] -> w643
              tunnel: [w654 w655] -> w642
              frame False {
              }
              frame True {
                n316 = call "串口读写 - WK.vi"("错误输入（无错误）"=w657, "写入设备"="TC2:TCSW=0\r" ("写入缓冲区"), "VISA输入"=w658) -> ("错误输出"=w656:errorcluster, "VISA输出"=w655:refnum<visa-resource-name>)  [unwired: 5 in, 2 out]
              }
            }
            n317 = VISA Close(VISA resource name=w642, error in (no error)=w643) -> (error out=w640:errorcluster)
          }
        }
        n318 = local write "打开串口"(w627) -> ()
        n319 = local write "温控开关 1"(w627) -> ()
        n320 = local write "温控开关 2"(w627) -> ()
        n321 = Bundle By Name(cluster=w620, "温控情况.打开串口"=w627, "开关信息.开关 1"=w627, "开关信息.开关 2"=w627, "开关信息.温控是否打开"=w627) -> (w628:T17)
        n322 = call <vilib>:"Add State(s) to Queue__JKI_lib_State_Machine.vi"("State(s) in (\"\")"=w632) -> ("States Out"=w631:string)  [unwired: 14 in]
      }
      frame "Macro: Stop" {
        n323 = call-poly <userlib>:"Build Message with Arguments++.vi"("States With Replace Token"="//Send Message to Other CSM Modules\nAPI: Stop -@ Acquisition - <1>\nAPI: Stop -@ Logging - <1>\n\nMacro: Close", "<1>"=w663) -> ("States"=w660:string)  [unwired: 13 in]
        n324 = call <vilib>:"Add State(s) to Queue__jki_lib_state_machine.vi"("State(s) in Front (\"\")"=w660, "State(s) in (\"\")"=w661) -> ("States Out"=w662:string)  [unwired: 13 in]
      }
      frame "Macro: Exit" {
        w670 = "//Permanent unregistrations\nAcquired Data@Acquisition - <1> >> Data: Update Indicators -><unregister>\nAcquired Data@Acquisition - <1> >> API: Log@Logging - <1> -><unregister>\n\n//Permanent unregistrations\nError Occurred@Acquisition - <1> >> Error Handler -><unregister>\nError Occurred@Logging - <1> >> Error Handler -><unregister>\n\n\n//Exit\nMacro: Exit-@Logging - <1>\nMacro: Exit-@Acquisition - <1>\n\nMacro: Close\n\nData: Cleanup\nExit"  # //Permanent unregistrations Acquired Data@Acquisition - <1> >> Data: Update Indicators -><unregister> Acquired Data@Acquisition - <1> >> API: Log@Logging - <1> -><unregister>  //Permanent unregistrations Error Occurred@Acquisition - <1> >> Error Handler -><unregister> Error Occurred@Logging - <1> >> Error Handler -><unregister>   //Exit Macro: Exit-@Logging - <1> Macro: Exit-@Acquisition - <1>  Macro: Close  Data: Cleanup Exit
        # "#CSM \"Macro: Exit\"\nExit Macro (This is called once, when the VI exits)"
        n325 = local write "温控循环功能"(FALSE ("值(信号)")) -> ()
        n326 = call-poly <userlib>:"Build Message with Arguments++.vi"("States With Replace Token"=w670, "<1>"=w671) -> ("States"=w668:string)  [unwired: 13 in]
        n327 = call <vilib>:"Add State(s) to Queue__JKI_lib_State_Machine.vi"("State(s) in Front (\"\")"=w668, "State(s) in (\"\")"=w673) -> ("States Out"=w672:string)  [unwired: 13 in]
      }
      frame "---------- Action ----------" {
        # "#CSM \"Category Seperator\"\nDo not put any code in this frame."
        n328 = call <vilib>:"Add State(s) to Queue__JKI_lib_State_Machine.vi"("State(s) in (\"\")"=w676) -> ("States Out"=w675:string)  [unwired: 14 in]
      }
      frame "Action: Power Output 1" {
        # "#CSM \"Internal State\"\nThis category is used for holding internal states"
        n329 = call "Convert API String Arguments to Data.vim"("Reference Type"=FALSE, "API String"=w686) -> ("Data"=w680:bool)  [unwired: 6 in, 1 out]
        n330 = Unbundle By Name(w683) -> ("基本信息.USB Port"=w692:refnum<visa-resource-name>)
        n331 = Boolean To (0,1)(Boolean=w680) -> (0, 1=w688:i16)
        n332 = Number To Decimal String(number=w688) -> (decimal integer string=w684:string)  [unwired: 1 in]
        n333 = local write "温控开关 1"(w680) -> ()
        n334 = Concatenate Strings("TC1:TCSW=" ("写入缓冲区"), w684, "\r" ("写入缓冲区")) -> (w689:string)
        n335 = call "串口读写 - WK.vi"("错误输入（无错误）"=w687, "写入设备"=w689, "VISA输入"=w692) -> ("错误输出"=w681:errorcluster)  [unwired: 5 in, 3 out]
        n336 = Bundle By Name(cluster=w683, "输出参数.输出状态 1.功率输出"=w688, "开关信息.开关 1"=w680) -> (w682:T17)
        n337 = call "Convert Data To API String Arguments.vim"("Data"=w680) -> ("API String"=w679:string)  [unwired: 7 in, 1 out]
        n338 = call <vilib>:"Build State String with Arguments__JKI_lib_State_Machine.vi"("Arguments (\"\")"=w679, "State"="Acq: ONOFF1") -> ("State with Arguments"=w677:string)  [unwired: 4 in]
        n339 = call <vilib>:"Add State(s) to Queue__JKI_lib_State_Machine.vi"("State(s) in Front (\"\")"=w677, "State(s) in (\"\")"=w694) -> ("States Out"=w693:string)  [unwired: 13 in]
      }
      frame "Action: Power Output 2" {
        # "#CSM \"Internal State\"\nThis category is used for holding internal states"
        n340 = Unbundle By Name(w701) -> ("基本信息.USB Port"=w710:refnum<visa-resource-name>)
        n341 = call "Convert API String Arguments to Data.vim"("Reference Type"=FALSE, "API String"=w704) -> ("Data"=w696:bool)  [unwired: 6 in, 1 out]
        n342 = Boolean To (0,1)(Boolean=w696) -> (0, 1=w706:i16)
        n343 = Number To Decimal String(number=w706) -> (decimal integer string=w702:string)  [unwired: 1 in]
        n344 = local write "温控开关 2"(w696) -> ()
        n345 = Concatenate Strings("TC2:TCSW=" ("写入缓冲区"), w702, "\r" ("写入缓冲区")) -> (w707:string)
        n346 = call "串口读写 - WK.vi"("错误输入（无错误）"=w705, "写入设备"=w707, "VISA输入"=w710) -> ("错误输出"=w699:errorcluster)  [unwired: 5 in, 3 out]
        n347 = Bundle By Name(cluster=w701, "输出参数.输出状态 2.功率输出"=w706, "开关信息.开关 2"=w696) -> (w700:T17)
        n348 = call "Convert Data To API String Arguments.vim"("Data"=w696) -> ("API String"=w698:string)  [unwired: 7 in, 1 out]
        n349 = call <vilib>:"Build State String with Arguments__JKI_lib_State_Machine.vi"("Arguments (\"\")"=w698, "State"="Acq: ONOFF2") -> ("State with Arguments"=w695:string)  [unwired: 4 in]
        n350 = call <vilib>:"Add State(s) to Queue__JKI_lib_State_Machine.vi"("State(s) in Front (\"\")"=w695, "State(s) in (\"\")"=w712) -> ("States Out"=w711:string)  [unwired: 13 in]
      }
      frame "Action: Change Temp 1" {
        n351 = Unbundle By Name(w729) -> ("基本信息.USB Port"=w735:refnum<visa-resource-name>)
        n352 = local read "过温 1"() -> (w723:T6)
        n353 = call "Convert API String Arguments to Data.vim"("Reference Type"=0.0, "API String"=w726) -> ("Data"=w721:dbl)  [unwired: 6 in, 1 out]
        n354 = Unbundle By Name(w723) -> ("最高设定温度"=w719:dbl, "最低设定温度"=w718:dbl)
        n355 = In Range and Coerce(upper limit=w719, x=w721, lower limit=w718) -> (coerced(x)=w720:dbl)  [unwired: 1 out]
        n356 = Add(x=w720, y=0.0) -> (x+y=w715:dbl)
        n357 = Number To Fractional String(number=w715, precision (6)=i16 2 ("精度(6)")) -> (F-format string=w731:string)  [unwired: 2 in]
        n358 = Concatenate Strings("TC1:TCADJUSTTEMP=" ("写入缓冲区"), w731, "\r" ("写入缓冲区")) -> (w732:string)
        n359 = call "串口读写 - WK.vi"("错误输入（无错误）"=w724, "写入设备"=w732, "VISA输入"=w735) -> ("错误输出"=w727:errorcluster)  [unwired: 5 in, 3 out]
        n360 = local write "温控温度 1"(w715) -> ()
        n361 = Bundle By Name(cluster=w729, "温控情况.温控温度 1"=w715) -> (w728:T17)
        n362 = call "Convert Data To API String Arguments.vim"("Data"=w715) -> ("API String"=w716:string)  [unwired: 7 in, 1 out]
        n363 = call-poly <userlib>:"Build Message with Arguments++.vi"("States With Replace Token"="API: Control Temp 1 >> <param> -@ Acquisition - <1>" ("State"), "<param>"=w716, "<1>"=w713) -> ("States"=w714:string)  [unwired: 12 in]
        n364 = call <vilib>:"Add State(s) to Queue__JKI_lib_State_Machine.vi"("State(s) in Front (\"\")"=w714, "State(s) in (\"\")"=w737) -> ("States Out"=w736:string)  [unwired: 13 in]
      }
      frame "Action: Change Temp 2" {
        # "#CSM \"Internal State\"\nThis category is used for holding internal states"
        n365 = Unbundle By Name(w746) -> ("设备信息.双通道设备？"=w740:bool, "基本信息.USB Port"=w747:refnum<visa-resource-name>)
        n366 = case shown="False" w740 {
          tunnel: w747 -> [_ w773]
          tunnel: [w752 w767] -> w744
          tunnel: w743 -> [_ w766]
          tunnel: w742 -> [w752 w764]
          tunnel: [25.0 ("Data") w755] -> w741
          tunnel: ["" ("States") w754] -> w739
          tunnel: w738 -> [_ w753]
          frame False {
          }
          frame True {
            n367 = local read "过温 2"() -> (w760:T6)
            n368 = Unbundle By Name(w760) -> ("最高设定温度"=w761:dbl, "最低设定温度"=w762:dbl)
            n369 = call "Convert API String Arguments to Data.vim"("Reference Type"=0.0, "API String"=w766) -> ("Data"=w758:dbl)  [unwired: 6 in, 1 out]
            n370 = In Range and Coerce(upper limit=w761, x=w758, lower limit=w762) -> (coerced(x)=w763:dbl)  [unwired: 1 out]
            n371 = Add(x=w763, y=0.0) -> (x+y=w755:dbl)
            n372 = Number To Fractional String(number=w755, precision (6)=i16 2 ("精度(6)")) -> (F-format string=w769:string)  [unwired: 2 in]
            n373 = Concatenate Strings("TC2:TCADJUSTTEMP=" ("写入缓冲区"), w769, "\r" ("写入缓冲区")) -> (w770:string)
            n374 = call "串口读写 - WK.vi"("错误输入（无错误）"=w764, "写入设备"=w770, "VISA输入"=w773) -> ("错误输出"=w767:errorcluster)  [unwired: 5 in, 3 out]
            n375 = call "Convert Data To API String Arguments.vim"("Data"=w755) -> ("API String"=w756:string)  [unwired: 7 in, 1 out]
            n376 = call-poly <userlib>:"Build Message with Arguments++.vi"("States With Replace Token"="API: Control Temp 1 >> <param> -@ Acquisition - <1>" ("State"), "<param>"=w756, "<1>"=w753) -> ("States"=w754:string)  [unwired: 12 in]
          }
        }
        n377 = local write "温控温度 2"(w741) -> ()
        n378 = Bundle By Name(cluster=w746, "温控情况.温控温度 2"=w741) -> (w745:T17)
        n379 = call <vilib>:"Add State(s) to Queue__JKI_lib_State_Machine.vi"("State(s) in Front (\"\")"=w739, "State(s) in (\"\")"=w749) -> ("States Out"=w748:string)  [unwired: 13 in]
      }
      frame "Action: Power Switch 1" {
        # "#CSM \"Internal State\"\nThis category is used for holding internal states"
        n380 = call "Convert API String Arguments to Data.vim"("Reference Type"=FALSE, "API String"=w781) -> ("Data"=w775:bool)  [unwired: 6 in, 1 out]
        n381 = Unbundle By Name(w778) -> ("基本信息.USB Port"=w786:refnum<visa-resource-name>)
        n382 = Boolean To (0,1)(Boolean=w775) -> (0, 1=w774:i16)
        n383 = Number To Decimal String(number=w774) -> (decimal integer string=w779:string)  [unwired: 1 in]
        n384 = local write "温控开关 1"(w775) -> ()
        n385 = Concatenate Strings("TC1:TCSW=" ("写入缓冲区"), w779, "\r" ("写入缓冲区")) -> (w783:string)
        n386 = call "串口读写 - WK.vi"("错误输入（无错误）"=w782, "写入设备"=w783, "VISA输入"=w786) -> ("错误输出"=w776:errorcluster)  [unwired: 5 in, 3 out]
        n387 = Bundle By Name(cluster=w778, "输出参数.输出状态 1.功率输出"=w774, "开关信息.开关 1"=w775) -> (w777:T17)
        n388 = property on="过压/过流 1" class="Clust (严格)"("DisabledEnum"=w774) -> ()  [unwired: 2 in, 2 out]
        n389 = property on="输出设置 1" class="Clust (严格)"("DisabledEnum"=w774) -> ()  [unwired: 2 in, 2 out]
        n390 = call <vilib>:"Add State(s) to Queue__JKI_lib_State_Machine.vi"("State(s) in (\"\")"=w788) -> ("States Out"=w787:string)  [unwired: 14 in]
      }
      frame "Action: Power Switch 2" {
        # "#CSM \"Internal State\"\nThis category is used for holding internal states"
        n391 = Unbundle By Name(w793) -> ("基本信息.USB Port"=w801:refnum<visa-resource-name>)
        n392 = call "Convert API String Arguments to Data.vim"("Reference Type"=FALSE, "API String"=w796) -> ("Data"=w790:bool)  [unwired: 6 in, 1 out]
        n393 = Boolean To (0,1)(Boolean=w790) -> (0, 1=w789:i16)
        n394 = Number To Decimal String(number=w789) -> (decimal integer string=w794:string)  [unwired: 1 in]
        n395 = local write "温控开关 2"(w790) -> ()
        n396 = Concatenate Strings("TC2:TCSW=" ("写入缓冲区"), w794, "\r" ("写入缓冲区")) -> (w798:string)
        n397 = call "串口读写 - WK.vi"("错误输入（无错误）"=w797, "写入设备"=w798, "VISA输入"=w801) -> ("错误输出"=w791:errorcluster)  [unwired: 5 in, 3 out]
        n398 = Bundle By Name(cluster=w793, "输出参数.输出状态 2.功率输出"=w789, "开关信息.开关 2"=w790) -> (w792:T17)
        n399 = property on="过压/过流 2" class="Clust (严格)"("DisabledEnum"=w789) -> ()  [unwired: 2 in, 2 out]
        n400 = property on="输出设置 2" class="Clust (严格)"("DisabledEnum"=w789) -> ()  [unwired: 2 in, 2 out]
        n401 = call <vilib>:"Add State(s) to Queue__JKI_lib_State_Machine.vi"("State(s) in (\"\")"=w803) -> ("States Out"=w802:string)  [unwired: 14 in]
      }
      frame "Action: Output Set 1" {
        w809 = "/" ("字符串")
        n402 = call "Convert API String Arguments to Data.vim"("Reference Type"=w809, "error in (no error)"=w805, "API String"=w811) -> ("error out"=w808:errorcluster, "Data"=w810:string)  [unwired: 5 in]
        n403 = Unbundle By Name(w807) -> ("基本信息.USB Port"=w822:refnum<visa-resource-name>)
        n404 = Match Pattern(string=w810, regular expression=w809) -> (before substring=w818:string, after substring=w816:string)  [unwired: 1 in, 2 out]
        n405 = Fract/Exp String To Number(string=w816) -> (number=w815:dbl)  [unwired: 3 in, 1 out]
        n406 = case shown="\"1\"" w818 {
          tunnel: ["TC1:TCMODE" ("写入缓冲区") "TC1:TCMAXV" ("写入缓冲区")] -> w817
          tunnel: w807 -> [w825 w829]
          tunnel: [w824 w828] -> w806
          tunnel: w815 -> [w823 w827]
          frame "1" {
            n407 = Bundle By Name(cluster=w825, "输出参数.输出设置 1.输出模式"=w823) -> (w824:T17)
          }
          frame "2", Default {
            n408 = Bundle By Name(cluster=w829, "输出参数.输出设置 1.最大输出电压"=w827) -> (w828:T17)
          }
        }
        n409 = Concatenate Strings(w817, "=" ("写入缓冲区"), w816, "\r" ("写入缓冲区")) -> (w819:string)
        n410 = call "串口读写 - WK.vi"("错误输入（无错误）"=w808, "是否保存?(F)"=FALSE ("是否保存？"), "写入设备"=w819, "VISA输入"=w822) -> ("错误输出"=w804:errorcluster)  [unwired: 4 in, 3 out]
        n411 = call <vilib>:"Add State(s) to Queue__JKI_lib_State_Machine.vi"("State(s) in (\"\")"=w812) -> ("States Out"=w813:string)  [unwired: 14 in]
      }
      frame "Action: Output Set 2" {
        w836 = "/" ("字符串")
        n412 = call "Convert API String Arguments to Data.vim"("Reference Type"=w836, "error in (no error)"=w832, "API String"=w838) -> ("error out"=w835:errorcluster, "Data"=w837:string)  [unwired: 5 in]
        n413 = Unbundle By Name(w834) -> ("基本信息.USB Port"=w849:refnum<visa-resource-name>)
        n414 = Match Pattern(string=w837, regular expression=w836) -> (before substring=w845:string, after substring=w843:string)  [unwired: 1 in, 2 out]
        n415 = Fract/Exp String To Number(string=w843) -> (number=w842:dbl)  [unwired: 3 in, 1 out]
        n416 = case shown="\"2\", 默认" w845 {
          tunnel: ["TC2:TCMODE" ("写入缓冲区") "TC2:TCMAXV" ("写入缓冲区")] -> w844
          tunnel: w834 -> [w852 w856]
          tunnel: [w851 w855] -> w833
          tunnel: w842 -> [w850 w854]
          frame "1" {
            n417 = Bundle By Name(cluster=w852, "输出参数.输出设置 2.输出模式"=w850) -> (w851:T17)
          }
          frame "2", Default {
            n418 = Bundle By Name(cluster=w856, "输出参数.输出设置 2.最大输出电压"=w854) -> (w855:T17)
          }
        }
        n419 = Concatenate Strings(w844, "=" ("写入缓冲区"), w843, "\r" ("写入缓冲区")) -> (w846:string)
        n420 = call "串口读写 - WK.vi"("错误输入（无错误）"=w835, "是否保存?(F)"=FALSE ("是否保存？"), "写入设备"=w846, "VISA输入"=w849) -> ("错误输出"=w831:errorcluster)  [unwired: 4 in, 3 out]
        n421 = call <vilib>:"Add State(s) to Queue__JKI_lib_State_Machine.vi"("State(s) in (\"\")"=w839) -> ("States Out"=w840:string)  [unwired: 14 in]
      }
      frame "Action: PID Set 1" {
        w866 = "/" ("字符串")
        n422 = call "Convert API String Arguments to Data.vim"("Reference Type"=w866, "error in (no error)"=w864, "API String"=w868) -> ("error out"=w865:errorcluster, "Data"=w867:string)  [unwired: 5 in]
        n423 = Unbundle By Name(w862) -> ("基本信息.USB Port"=w876:refnum<visa-resource-name>)
        n424 = Match Pattern(string=w867, regular expression=w866) -> (before substring=w860:string, after substring=w872:string)  [unwired: 1 in, 2 out]
        n425 = Fract/Exp String To Number(string=w872) -> (number=w861:dbl)  [unwired: 3 in, 1 out]
        n426 = case shown="\"32\"" w860 {
          tunnel: ["" ("写入缓冲区") "TC1:TCPIDTYPE" ("写入缓冲区") "TC1:TCP" ("写入缓冲区") "TC1:TCTI" ("写入缓冲区") "TC1:TCTD" ("写入缓冲区") "TC1:TCCTRLINTERVAL" ("写入缓冲区") "TC1:TCPIDCAL" ("写入缓冲区")] -> w859
          tunnel: w862 -> [w878 w881 w885 w889 w893 w897 w901]
          tunnel: [w878 w880 w884 w888 w892 w896 w900] -> w858
          tunnel: w861 -> [_ w879 w883 w887 w891 w895 w899]
          frame "0", Default {
          }
          frame "1" {
            n427 = Bundle By Name(cluster=w881, "输出参数.PID 1.PID类型"=w879) -> (w880:T17)
          }
          frame "2" {
            n428 = Bundle By Name(cluster=w885, "输出参数.PID 1.P"=w883) -> (w884:T17)
          }
          frame "4" {
            n429 = Bundle By Name(cluster=w889, "输出参数.PID 1.I"=w887) -> (w888:T17)
          }
          frame "8" {
            n430 = Bundle By Name(cluster=w893, "输出参数.PID 1.D"=w891) -> (w892:T17)
          }
          frame "16" {
            n431 = Bundle By Name(cluster=w897, "输出参数.PID 1.PID控制间隔"=w895) -> (w896:T17)
          }
          frame "32" {
            n432 = Bundle By Name(cluster=w901, "输出参数.PID 1.PID计算方法"=w899) -> (w900:T17)
          }
        }
        n433 = Concatenate Strings(w859, "=" ("写入缓冲区"), w872, "\r" ("写入缓冲区")) -> (w873:string)
        n434 = call "串口读写 - WK.vi"("错误输入（无错误）"=w865, "是否保存?(F)"=FALSE ("是否保存？"), "写入设备"=w873, "VISA输入"=w876) -> ("错误输出"=w863:errorcluster)  [unwired: 4 in, 3 out]
        n435 = call <vilib>:"Add State(s) to Queue__JKI_lib_State_Machine.vi"("State(s) in (\"\")"=w869) -> ("States Out"=w870:string)  [unwired: 14 in]
      }
      frame "Action: PID Set 2" {
        w911 = "/" ("字符串")
        n436 = call "Convert API String Arguments to Data.vim"("Reference Type"=w911, "error in (no error)"=w909, "API String"=w913) -> ("error out"=w910:errorcluster, "Data"=w912:string)  [unwired: 5 in]
        n437 = Unbundle By Name(w905) -> ("基本信息.USB Port"=w921:refnum<visa-resource-name>)
        n438 = Match Pattern(string=w912, regular expression=w911) -> (before substring=w906:string, after substring=w917:string)  [unwired: 1 in, 2 out]
        n439 = Fract/Exp String To Number(string=w917) -> (number=w907:dbl)  [unwired: 3 in, 1 out]
        n440 = case shown="\"0\", 默认" w906 {
          tunnel: ["" ("写入缓冲区") "TC2:TCPIDTYPE" ("写入缓冲区") "TC2:TCP" ("写入缓冲区") "TC2:TCTI" ("写入缓冲区") "TC2:TCTD" ("写入缓冲区") "TC2:TCCTRLINTERVAL" ("写入缓冲区") "TC2:TCPIDCAL" ("写入缓冲区")] -> w903
          tunnel: w905 -> [w923 w926 w930 w934 w938 w942 w946]
          tunnel: [w923 w925 w929 w933 w937 w941 w945] -> w904
          tunnel: w907 -> [_ w924 w928 w932 w936 w940 w944]
          frame "0", Default {
          }
          frame "1" {
            n441 = Bundle By Name(cluster=w926, "输出参数.PID 2.PID类型"=w924) -> (w925:T17)
          }
          frame "2" {
            n442 = Bundle By Name(cluster=w930, "输出参数.PID 2.P"=w928) -> (w929:T17)
          }
          frame "4" {
            n443 = Bundle By Name(cluster=w934, "输出参数.PID 2.I"=w932) -> (w933:T17)
          }
          frame "8" {
            n444 = Bundle By Name(cluster=w938, "输出参数.PID 2.D"=w936) -> (w937:T17)
          }
          frame "16" {
            n445 = Bundle By Name(cluster=w942, "输出参数.PID 2.PID控制间隔"=w940) -> (w941:T17)
          }
          frame "32" {
            n446 = Bundle By Name(cluster=w946, "输出参数.PID 2.PID计算方法"=w944) -> (w945:T17)
          }
        }
        n447 = Concatenate Strings(w903, "=" ("写入缓冲区"), w917, "\r" ("写入缓冲区")) -> (w918:string)
        n448 = call "串口读写 - WK.vi"("错误输入（无错误）"=w910, "是否保存?(F)"=FALSE ("是否保存？"), "写入设备"=w918, "VISA输入"=w921) -> ("错误输出"=w908:errorcluster)  [unwired: 4 in, 3 out]
        n449 = call <vilib>:"Add State(s) to Queue__JKI_lib_State_Machine.vi"("State(s) in (\"\")"=w914) -> ("States Out"=w915:string)  [unwired: 14 in]
      }
      frame "Action: OTP Set 1" {
        w956 = "/" ("字符串")
        n450 = call "Convert API String Arguments to Data.vim"("Reference Type"=w956, "error in (no error)"=w954, "API String"=w958) -> ("error out"=w955:errorcluster, "Data"=w957:string)  [unwired: 5 in]
        n451 = Unbundle By Name(w951) -> ("基本信息.USB Port"=w966:refnum<visa-resource-name>)
        n452 = Match Pattern(string=w957, regular expression=w956) -> (before substring=w952:string, after substring=w962:string)  [unwired: 1 in, 2 out]
        n453 = Fract/Exp String To Number(string=w962) -> (number=w950:dbl)  [unwired: 3 in, 1 out]
        n454 = case shown="\"1\"" w952 {
          tunnel: ["" ("写入缓冲区") "TC1:TCOTPE" ("写入缓冲区") "TC1:TCOTPLT" ("写入缓冲区") "TC1:TCOTPHT" ("写入缓冲区") "TC1:TCMINSETTEMP" ("写入缓冲区") "TC1:TCMAXSETTEMP" ("写入缓冲区") "TC1:TCRAMPSPEED" ("写入缓冲区")] -> w948
          tunnel: w951 -> [w968 w972 w976 w980 w984 w988 w992]
          tunnel: [w968 w971 w975 w979 w983 w987 w991] -> w949
          tunnel: w950 -> [_ w970 w974 w978 w982 w986 w990]
          frame "0", Default {
          }
          frame "1" {
            n455 = Not Equal To 0?(x=w970) -> (x != 0?=w969:bool)
            n456 = Bundle By Name(cluster=w972, "保护.过温 1.过温保护开关"=w969) -> (w971:T17)
          }
          frame "2" {
            n457 = Bundle By Name(cluster=w976, "保护.过温 1.过温保护低阈值"=w974) -> (w975:T17)
          }
          frame "4" {
            n458 = Bundle By Name(cluster=w980, "保护.过温 1.过温保护高阈值"=w978) -> (w979:T17)
          }
          frame "8" {
            n459 = Bundle By Name(cluster=w984, "保护.过温 1.最低设定温度"=w982) -> (w983:T17)
          }
          frame "16" {
            n460 = Bundle By Name(cluster=w988, "保护.过温 1.最高设定温度"=w986) -> (w987:T17)
          }
          frame "32" {
            n461 = Bundle By Name(cluster=w992, "保护.过温 1.温度限速"=w990) -> (w991:T17)
          }
        }
        n462 = Concatenate Strings(w948, "=" ("写入缓冲区"), w962, "\r" ("写入缓冲区")) -> (w963:string)
        n463 = call "串口读写 - WK.vi"("错误输入（无错误）"=w955, "是否保存?(F)"=FALSE ("是否保存？"), "写入设备"=w963, "VISA输入"=w966) -> ("错误输出"=w953:errorcluster)  [unwired: 4 in, 3 out]
        n464 = call <vilib>:"Add State(s) to Queue__JKI_lib_State_Machine.vi"("State(s) in (\"\")"=w959) -> ("States Out"=w960:string)  [unwired: 14 in]
      }
      frame "Action: OTP Set 2" {
        w1002 = "/" ("字符串")
        n465 = call "Convert API String Arguments to Data.vim"("Reference Type"=w1002, "error in (no error)"=w1000, "API String"=w1004) -> ("error out"=w1001:errorcluster, "Data"=w1003:string)  [unwired: 5 in]
        n466 = Unbundle By Name(w998) -> ("基本信息.USB Port"=w1012:refnum<visa-resource-name>)
        n467 = Match Pattern(string=w1003, regular expression=w1002) -> (before substring=w997:string, after substring=w1008:string)  [unwired: 1 in, 2 out]
        n468 = Fract/Exp String To Number(string=w1008) -> (number=w996:dbl)  [unwired: 3 in, 1 out]
        n469 = case shown="\"0\", 默认" w997 {
          tunnel: ["" ("写入缓冲区") "TC2:TCOTPE" ("写入缓冲区") "TC2:TCOTPLT" ("写入缓冲区") "TC2:TCOTPHT" ("写入缓冲区") "TC2:TCMINSETTEMP" ("写入缓冲区") "TC2:TCMAXSETTEMP" ("写入缓冲区") "TC2:TCRAMPSPEED" ("写入缓冲区")] -> w995
          tunnel: w998 -> [w1014 w1018 w1022 w1026 w1030 w1034 w1038]
          tunnel: [w1014 w1017 w1021 w1025 w1029 w1033 w1037] -> w994
          tunnel: w996 -> [_ w1016 w1020 w1024 w1028 w1032 w1036]
          frame "0", Default {
          }
          frame "1" {
            n470 = Not Equal To 0?(x=w1016) -> (x != 0?=w1015:bool)
            n471 = Bundle By Name(cluster=w1018, "保护.过温 2.过温保护开关"=w1015) -> (w1017:T17)
          }
          frame "2" {
            n472 = Bundle By Name(cluster=w1022, "保护.过温 2.过温保护低阈值"=w1020) -> (w1021:T17)
          }
          frame "4" {
            n473 = Bundle By Name(cluster=w1026, "保护.过温 2.过温保护高阈值"=w1024) -> (w1025:T17)
          }
          frame "8" {
            n474 = Bundle By Name(cluster=w1030, "保护.过温 2.最低设定温度"=w1028) -> (w1029:T17)
          }
          frame "16" {
            n475 = Bundle By Name(cluster=w1034, "保护.过温 2.最高设定温度"=w1032) -> (w1033:T17)
          }
          frame "32" {
            n476 = Bundle By Name(cluster=w1038, "保护.过温 2.温度限速"=w1036) -> (w1037:T17)
          }
        }
        n477 = Concatenate Strings(w995, "=" ("写入缓冲区"), w1008, "\r" ("写入缓冲区")) -> (w1009:string)
        n478 = call "串口读写 - WK.vi"("错误输入（无错误）"=w1001, "是否保存?(F)"=FALSE ("是否保存？"), "写入设备"=w1009, "VISA输入"=w1012) -> ("错误输出"=w999:errorcluster)  [unwired: 4 in, 3 out]
        n479 = call <vilib>:"Add State(s) to Queue__JKI_lib_State_Machine.vi"("State(s) in (\"\")"=w1005) -> ("States Out"=w1006:string)  [unwired: 14 in]
      }
      frame "Action: OVP Set 1" {
        w1048 = "/" ("字符串")
        n480 = call "Convert API String Arguments to Data.vim"("Reference Type"=w1048, "error in (no error)"=w1046, "API String"=w1050) -> ("error out"=w1047:errorcluster, "Data"=w1049:string)  [unwired: 5 in]
        n481 = Unbundle By Name(w1042) -> ("基本信息.USB Port"=w1058:refnum<visa-resource-name>)
        n482 = Match Pattern(string=w1049, regular expression=w1048) -> (before substring=w1041:string, after substring=w1054:string)  [unwired: 1 in, 2 out]
        n483 = Fract/Exp String To Number(string=w1054) -> (number=w1040:dbl)  [unwired: 3 in, 1 out]
        n484 = case shown="\"2\"" w1041 {
          tunnel: ["" ("写入缓冲区") "TC1:TCADJUSTOVPV" ("写入缓冲区") "TC1:TCADJUSTOCPC" ("写入缓冲区")] -> w1044
          tunnel: w1042 -> [w1060 w1063 w1067]
          tunnel: [w1060 w1062 w1066] -> w1043
          tunnel: w1040 -> [_ w1061 w1065]
          frame "0", Default {
          }
          frame "1" {
            n485 = Bundle By Name(cluster=w1063, "保护.过压/过流 1.过压保护阈值"=w1061) -> (w1062:T17)
          }
          frame "2" {
            n486 = Bundle By Name(cluster=w1067, "保护.过压/过流 1.过流保护阈值"=w1065) -> (w1066:T17)
          }
        }
        n487 = Concatenate Strings(w1044, "=" ("写入缓冲区"), w1054, "\r" ("写入缓冲区")) -> (w1055:string)
        n488 = call "串口读写 - WK.vi"("错误输入（无错误）"=w1047, "是否保存?(F)"=FALSE ("是否保存？"), "写入设备"=w1055, "VISA输入"=w1058) -> ("错误输出"=w1045:errorcluster)  [unwired: 4 in, 3 out]
        n489 = call <vilib>:"Add State(s) to Queue__JKI_lib_State_Machine.vi"("State(s) in (\"\")"=w1051) -> ("States Out"=w1052:string)  [unwired: 14 in]
      }
      frame "Action: OVP Set 2" {
        w1077 = "/" ("字符串")
        n490 = call "Convert API String Arguments to Data.vim"("Reference Type"=w1077, "error in (no error)"=w1075, "API String"=w1079) -> ("error out"=w1076:errorcluster, "Data"=w1078:string)  [unwired: 5 in]
        n491 = Unbundle By Name(w1071) -> ("基本信息.USB Port"=w1087:refnum<visa-resource-name>)
        n492 = Match Pattern(string=w1078, regular expression=w1077) -> (before substring=w1070:string, after substring=w1083:string)  [unwired: 1 in, 2 out]
        n493 = Fract/Exp String To Number(string=w1083) -> (number=w1069:dbl)  [unwired: 3 in, 1 out]
        n494 = case shown="\"1\"" w1070 {
          tunnel: ["" ("写入缓冲区") "TC2:TCADJUSTOVPV" ("写入缓冲区") "TC2:TCADJUSTOCPC" ("写入缓冲区")] -> w1073
          tunnel: w1071 -> [w1089 w1092 w1096]
          tunnel: [w1089 w1091 w1095] -> w1072
          tunnel: w1069 -> [_ w1090 w1094]
          frame "0", Default {
          }
          frame "1" {
            n495 = Bundle By Name(cluster=w1092, "保护.过压/过流 2.过压保护阈值"=w1090) -> (w1091:T17)
          }
          frame "2" {
            n496 = Bundle By Name(cluster=w1096, "保护.过压/过流 2.过流保护阈值"=w1094) -> (w1095:T17)
          }
        }
        n497 = Concatenate Strings(w1073, "=" ("写入缓冲区"), w1083, "\r" ("写入缓冲区")) -> (w1084:string)
        n498 = call "串口读写 - WK.vi"("错误输入（无错误）"=w1076, "是否保存?(F)"=FALSE ("是否保存？"), "写入设备"=w1084, "VISA输入"=w1087) -> ("错误输出"=w1074:errorcluster)  [unwired: 4 in, 3 out]
        n499 = call <vilib>:"Add State(s) to Queue__JKI_lib_State_Machine.vi"("State(s) in (\"\")"=w1080) -> ("States Out"=w1081:string)  [unwired: 14 in]
      }
      frame "---------- Acq ----------" {
        # "#CSM \"Category Seperator\"\nDo not put any code in this frame."
      }
      frame "Acq: Fast Mode" {
        n500 = call "Convert API String Arguments to Data.vim"("Reference Type"=FALSE ("Fast Mode"), "API String"=w1104) -> ("Data"=w1101:bool)  [unwired: 6 in, 1 out]
        n501 = call-poly <userlib>:"Build Message with Arguments++.vi"("States With Replace Token"="API: Fast Mode >> <param> ->| Acquisition - <1>" ("State"), "<param>"=w1104, "<1>"=w1108) -> ("States"=w1105:string)  [unwired: 12 in]
        n502 = call <vilib>:"Add State(s) to Queue__JKI_lib_State_Machine.vi"("State(s) in Front (\"\")"=w1105, "State(s) in (\"\")"=w1106) -> ("States Out"=w1107:string)  [unwired: 13 in]
        n503 = Bundle By Name(cluster=w1102, "其他.Fast Mode?"=w1101) -> (w1100:T17)
      }
      frame "Acq: ONOFF1" {
        n504 = call-poly <userlib>:"Build Message with Arguments++.vi"("States With Replace Token"="API: ONOFF1 >> <param> ->| Acquisition - <1>" ("State"), "<param>"=w1115, "<1>"=w1114) -> ("States"=w1111:string)  [unwired: 12 in]
        n505 = call <vilib>:"Add State(s) to Queue__JKI_lib_State_Machine.vi"("State(s) in Front (\"\")"=w1111, "State(s) in (\"\")"=w1112) -> ("States Out"=w1113:string)  [unwired: 13 in]
      }
      frame "Acq: ONOFF2" {
        n506 = call-poly <userlib>:"Build Message with Arguments++.vi"("States With Replace Token"="API: ONOFF2 >> <param> ->| Acquisition - <1>" ("State"), "<param>"=w1123, "<1>"=w1122) -> ("States"=w1119:string)  [unwired: 12 in]
        n507 = call <vilib>:"Add State(s) to Queue__JKI_lib_State_Machine.vi"("State(s) in Front (\"\")"=w1119, "State(s) in (\"\")"=w1120) -> ("States Out"=w1121:string)  [unwired: 13 in]
      }
      frame "Acq: Sample Interval" {
        n508 = call-poly <userlib>:"Build Message with Arguments++.vi"("States With Replace Token"="API: Sample Interval >> <param> ->| Acquisition - <1>" ("State"), "<param>"=w1130, "<1>"=w1135) -> ("States"=w1132:string)  [unwired: 12 in]
        n509 = call "Convert API String Arguments to Data.vim"("Reference Type"=0.0, "API String"=w1130) -> ("Data"=w1129:dbl)  [unwired: 6 in, 1 out]
        n510 = Bundle By Name(cluster=w1131, "基本信息.采集间隔(s)"=w1129) -> (w1127:T17)
        n511 = call <vilib>:"Add State(s) to Queue__JKI_lib_State_Machine.vi"("State(s) in Front (\"\")"=w1132, "State(s) in (\"\")"=w1133) -> ("States Out"=w1134:string)  [unwired: 13 in]
      }
      frame "---------- Repeat ----------" {
        # "#CSM \"Internal State\"\nThis category is used for holding internal states"
        n512 = call <vilib>:"Add State(s) to Queue__JKI_lib_State_Machine.vi"("State(s) in (\"\")"=w1140) -> ("States Out"=w1139:string)  [unwired: 14 in]
      }
      frame "Repeat: Enable" {
        w1142 = T23 [{"控制温度"=25.0, "时长(s)"=60.0, "进度"=1.000390362739563, "温控开关"=FALSE}, {"控制温度"=26.0, "时长(s)"=60.0, "进度"=1.0013926823933919, "温控开关"=TRUE}, {"控制温度"=25.0, "时长(s)"=60.0, "进度"=1.0006222248077392, "温控开关"=FALSE}, {"控制温度"=26.0, "时长(s)"=60.0, "进度"=0.6612281163533529, "温控开关"=TRUE}]  # 步骤
        # "注意不是簇，是簇的数组，所以不可以用"
        # "#CSM \"Internal State\"\nThis category is used for holding internal states"
        n513 = call "CSM - Read Configuration Variable.vim"("Section Name (\"\" as Default)"=w1141, "Configuration Prototype (Cluster Prefered)"=w1142) -> ("Configuration"=w1143:T23)  [unwired: 6 in, 1 out]
        n514 = Concatenate Strings("Repeat - " ("Name(\"\" to use uuid)"), w1141) -> (w1148:string)
        n515 = control-ref of="子面板-Repeat"() -> (w1151:refnum<vi>)
        n516 = vi-ref "UI-温度控制.lvlib:Repeat.lvlib:Repeat.vi"() -> (w1150:refnum<vi>)
        n517 = call "Convert Data To API String Arguments.vim"("Data"=w1143) -> ("API String"=w1144:string)  [unwired: 7 in, 1 out]
        n518 = disable-structure shown="禁用" {
          frame Disabled {
            n519 = call "CSM - Read Cluster Elements From Session.vim"() -> ()  [unwired: 8 in, 2 out]
          }
          frame Enabled {
          }
        }
        n520 = call "打开引用.vi"("引用"=w1151, "CSM Name"=w1148, "VI"=w1150) -> ("错误输出"=w1146:errorcluster)  [unwired: 7 in, 1 out]
        n521 = flat-sequence {
          tunnel: [w1159] -> w1147
          tunnel: w1141 -> [w1157]
          tunnel: w1146 -> [_]
          tunnel: w1144 -> [w1154]
          frame #0 {
            w1161 = "Error Occurred@Repeat - <1> >> Error Handler -><register>\nRepeat Changed@Repeat - <1> >> Save Repeat -><register>"  # Error Occurred@Repeat - <1> >> Error Handler -><register> Repeat Changed@Repeat - <1> >> Save Repeat -><register>
            n522 = Wait (ms)(milliseconds to wait=u32 100 ("等待时间（毫秒）")) -> ()  [unwired: 1 out]
            n523 = call <vilib>:"Add State(s) to Queue__JKI_lib_State_Machine.vi"("State(s) in Front (\"\")"=w1161, "State(s) in (\"\")"="API: CSM Name  >> <1> ->| Repeat - <1> ", "State(s) at Back (\"\")"="API: INI Read  >> <param> ->| Repeat - <1> ") -> ("States Out"=w1160:string)  [unwired: 12 in]
            n524 = call-poly <userlib>:"Build Message with Arguments++.vi"("States With Replace Token"=w1160, "<param>"=w1154, "<1>"=w1157) -> ("States"=w1159:string)  [unwired: 12 in]
          }
        }
        n525 = call <vilib>:"Add State(s) to Queue__JKI_lib_State_Machine.vi"("State(s) in Front (\"\")"=w1147, "State(s) in (\"\")"=w1153) -> ("States Out"=w1152:string)  [unwired: 13 in]
      }
      frame "Save Repeat" {
        w1165 = T23 [{"控制温度"=25.0, "时长(s)"=60.0, "进度"=1.000390362739563, "温控开关"=FALSE}, {"控制温度"=26.0, "时长(s)"=60.0, "进度"=1.0013926823933919, "温控开关"=TRUE}, {"控制温度"=25.0, "时长(s)"=60.0, "进度"=1.0006222248077392, "温控开关"=FALSE}, {"控制温度"=26.0, "时长(s)"=60.0, "进度"=0.6612281163533529, "温控开关"=TRUE}]  # 循环步骤
        n526 = call "Convert API String Arguments to Data.vim"("Reference Type"=w1165, "API String"=w1164) -> ("Data"=w1163:T23)  [unwired: 6 in, 1 out]
        n527 = call "CSM - Write Configuration Variable.vim"("Section Name (\"\" as Default)"=w1162, "Configuration"=w1163) -> ()  [unwired: 6 in, 2 out]
        n528 = call <vilib>:"Add State(s) to Queue__jki_lib_state_machine.vi"("State(s) in (\"\")"=w1166) -> ("States Out"=w1167:string)  [unwired: 14 in]
      }
      frame "Repeat: Disable" {
        w1174 = "Error Occurred@Repeat - <1> >> Error Handler -><unregister>\nRepeat Changed@Repeat - <1> >> Save Repeat -><unregister>"  # Error Occurred@Repeat - <1> >> Error Handler -><unregister> Repeat Changed@Repeat - <1> >> Save Repeat -><unregister>
        # "#CSM \"Internal State\"\nThis category is used for holding internal states"
        n529 = call <vilib>:"Add State(s) to Queue__JKI_lib_State_Machine.vi"("State(s) in Front (\"\")"=w1174, "State(s) in (\"\")"="Macro: Exit-@Repeat - <1>", "State(s) at Back (\"\")"="Repeat: Remove" ("State(s) at Back (\"\")")) -> ("States Out"=w1172:string)  [unwired: 12 in]
        n530 = call-poly <userlib>:"Build Message with Arguments++.vi"("States With Replace Token"=w1172, "<1>"=w1175) -> ("States"=w1171:string)  [unwired: 13 in]
        n531 = call <vilib>:"Add State(s) to Queue__JKI_lib_State_Machine.vi"("State(s) in Front (\"\")"=w1171, "State(s) in (\"\")"=w1178) -> ("States Out"=w1177:string)  [unwired: 13 in]
      }
      frame "Repeat: Remove" {
        n532 = control-ref of="子面板-Repeat"() -> (w1181:refnum<vi>)
        n533 = invoke class="SubPnl" method="Remove VI"(reference=w1181) -> (error out=w1179:errorcluster)  [unwired: 2 in, 2 out]
        n534 = vi-ref "UI-温度控制.lvlib:Repeat.lvlib:Repeat.vi"() -> (w1180:refnum<vi>)
        n535 = call "关闭引用.vi"("错误输入（无错误）"=w1179, "引用"=w1180) -> ()  [unwired: 9 in, 1 out]
      }
    }
    n536 = Unbundle By Name(w33) -> ("其他.子程序？"=w32:bool)
    n537 = call "State Delete.vi"("Delete?(F)"=w32, "CSM name to delete"=string[] ["Logging"], "State In"=w36) -> ("State Out"=w35:string)  [unwired: 8 in]
  }
  n538 = while {
    shift-right: [w1195] -> _
    shift-left: enum16{"Idle", "Initialize", "Exit"}."Initialize" -> [w1196]
    tunnel: "CSM Name" -> [w1193]
    shift-right: [w1191] -> _
    shift-left: w9 -> [w1192]
    shift-right: [w1189] -> _
    shift-left: -1 -> [w1190]
    shift-right: [w1188] -> _
    shift-left: _ -> [w1187]
    shift-right: [w1186] -> _
    shift-left: _ -> [w1185]
    stop <- w1194 stop-if-true
    n539 = case shown="\"Idle\", 默认" w1196 {
      tunnel: [enum16{"Idle", "Initialize", "Exit"}."Idle" w1214 enum16{"Idle", "Initialize", "Exit"}."Exit"] -> w1195
      tunnel: [_ _ TRUE] -> w1194
      tunnel: w1193 -> [w1200 w1213 _]
      tunnel: w1192 -> [w1203 w1211 w1623]
      tunnel: [w1203 w1212 w1623] -> w1191
      tunnel: w1190 -> [_ w1209 _]
      tunnel: [-1 w1210 _] -> w1189
      tunnel: [w1199 w1207 _] -> w1188
      tunnel: w1187 -> [_ w1208 w1622]
      tunnel: [w1197 w1205 w1620] -> w1186
      tunnel: w1185 -> [_ w1206 w1620]
      frame "Initialize" {
        w1198 = FALSE  # your data
        n540 = call <userlib>:"CSM - Module Exit Event.vi"("Name (\"\" to Use UUID) In"=w1200) -> ("CSM Exit Event"=w1201:refnum<user-event>)  [unwired: 8 in, 2 out]
        n541 = register-events(w1201) -> (reference out=w1199:refnum<event-registration>)  [unwired: 2 in, 1 out]
        n542 = Bundle("your data"=w1198) -> (w1197:cluster{"your data":bool})  [unwired: 1 in]
      }
      frame "Idle", Default {
        n543 = event shown="[12] \"上限 1\", \"下限 1\", \"上限 2\", \"下限 2\": 值改变" {
          selector: w1208 -> [_ _ _ _ _ _ _ _ _ _ _ _ _ _ _ _ _ _ _ _ _ _ _ _ _ _]
          dyn-events: [_ _ _ _ _ _ _ _ _ _ _ _ _ _ _ _ _ _ _ _ _ _ _ _ _ _] -> w1207
          timeout: w1209 -> [_ _ _ _ _ _ _ _ _ _ _ _ _ _ _ _ _ _ _ _ _ _ _ _ _ _]
          tunnel: [_ w1221 enum16{"Idle", "Initialize", "Exit"}."Exit" _ _ _ _ _ _ _ _ _ _ _ _ _ _ _ _ _ _ _ _ _ _ _] -> w1214
          tunnel: w1213 -> [w1216 w1226 _ _ _ _ _ _ _ _ _ _ _ _ _ _ _ _ _ _ _ _ _ _ _ _]
          tunnel: w1211 -> [w1219 _ w1236 w1243 w1251 w1259 w1272 w1287 w1299 w1311 w1313 w1324 w1328 w1335 w1342 w1349 w1356 w1372 w1404 w1427 w1456 w1485 w1515 w1549 w1582 w1612]
          tunnel: [w1217 w1225 w1236 w1242 w1247 w1258 w1271 w1286 w1298 w1310 w1314 w1325 w1329 w1336 w1343 w1350 w1357 w1373 w1405 w1428 w1457 w1486 w1516 w1550 w1583 w1613] -> w1212
          tunnel: [-1 _ _ _ _ _ _ _ _ _ _ _ _ _ _ _ _ _ _ _ _ _ _ _ _ _] -> w1210
          tunnel: w1206 -> [w1215 w1224 w1234 w1244 w1252 w1260 w1273 w1288 w1300 w1312 w1320 w1326 w1330 w1337 w1344 w1351 w1358 w1378 w1410 w1438 w1467 w1496 w1526 w1560 w1593 w1614]
          tunnel: [w1215 w1224 w1234 w1244 w1252 w1260 w1273 w1288 w1300 w1312 w1320 w1326 w1330 w1337 w1344 w1351 w1358 w1378 w1410 w1438 w1467 w1496 w1526 w1560 w1593 w1614] -> w1205
          event Timeout {
            n544 = event-data() -> ()  [unwired: 1 in, 3 out]
            n545 = call-poly <userlib>:"CSM - Filter JKISM String Queue.vi"("States In"=w1219) -> ("States Out"=w1218:string)  [unwired: 14 in]
            n546 = call <userlib>:"CSM - Forward UI Operations to CSM.vi"("Name (\"\" to Use UUID)"=w1216, "State(s) In (\"\")"=w1218) -> ("States Out"=w1217:string)  [unwired: 8 in, 1 out]
          }
          event Panel Close? {
            # "#CSM \nIf you use this as the topmost VI\nDo not set it to FALSE"
            n547 = event-data() -> ()  [unwired: 1 in, 1 out]
            n548 = Two Button Dialog(message="确定关闭程序？" ("消息")) -> (T button?=w1222:bool)  [unwired: 2 in]
            n549 = case shown="False" w1222 {
              tunnel: w1226 -> [w1229 w1232]
              tunnel: [w1229 w1231] -> w1225
              tunnel: [enum16{"Idle", "Initialize", "Exit"}."Idle" enum16{"Idle", "Initialize", "Exit"}."Exit"] -> w1221
              frame False {
              }
              frame True {
                n550 = call <userlib>:"CSM - Forward UI Operations to CSM.vi"("Name (\"\" to Use UUID)"=w1232, "State(s) In (\"\")"="Macro: Exit" ("State")) -> ("States Out"=w1231:string)  [unwired: 8 in, 1 out]
              }
            }
            n551 = event-data("Discard?"=TRUE) -> ()  [unwired: 1 in, 1 out]
          }
          event User Event {
            n552 = event-data() -> ()  [unwired: 1 in, 1 out]
          }
          event "停止": Value Change {
            n553 = event-data() -> ()  [unwired: 1 in, 1 out]
            n554 = Two Button Dialog(message="确定停止程序？" ("消息")) -> (T button?=w1239:bool)  [unwired: 2 in]
            n555 = Select(t="Macro: Exit" ("State(s) in Front (\"\")"), s=w1239, f="") -> (s? t:f=w1237:string)
            n556 = call <vilib>:"Add State(s) to Queue__JKI_lib_State_Machine.vi"("State(s) in Front (\"\")"=w1237, "State(s) in (\"\")"=w1243) -> ("States Out"=w1242:string)  [unwired: 13 in]
          }
          event "打开串口": Value Change {
            n557 = event-data() -> ()  [unwired: 1 in, 1 out]
            n558 = call-poly <userlib>:"Add State(s) to Queue By BOOL++.vi"("FALSE (\"\")"="Macro: Stop" ("State(s) in Front (\"\")"), "TRUE (\"\")"="Macro: Start" ("State(s) in Front (\"\")"), "High Priority? (F)"=TRUE, "Condition"="打开串口", "State Queue (\"\")"=w1251) -> ("Remaining States"=w1247:string)  [unwired: 6 in]
            n559 = local write "温控-错误输出"(errorcluster {"status"=FALSE, "code"=0, "source"=""} ("错误常量")) -> ()
          }
          event "温控开关 1": Value Change {
            n560 = event-data() -> ("OldVal"=w1254:bool, "NewVal"=w1255:bool)  [unwired: 1 in]
            n561 = Not Equal?(x=w1254, y=w1255) -> (x != y?=w1253:bool)
            n562 = case shown="True" w1253 {
              tunnel: ["" ("State with Arguments") w1263] -> w1257
              tunnel: "温控开关 1" -> [_ w1262]
              frame False {
              }
              frame True {
                n563 = call "Convert Data To API String Arguments.vim"("Data"=w1262) -> ("API String"=w1265:string)  [unwired: 7 in, 1 out]
                n564 = call <vilib>:"Build State String with Arguments__JKI_lib_State_Machine.vi"("Arguments (\"\")"=w1265, "State"="Action: Power Output 1" ("State(s) in Front (\"\")")) -> ("State with Arguments"=w1263:string)  [unwired: 4 in]
              }
            }
            n565 = call <vilib>:"Add State(s) to Queue__JKI_lib_State_Machine.vi"("State(s) in Front (\"\")"=w1257, "State(s) in (\"\")"=w1259) -> ("States Out"=w1258:string)  [unwired: 13 in]
          }
          event "温控开关 2": Value Change {
            n566 = event-data() -> ("OldVal"=w1267:bool, "NewVal"=w1268:bool)  [unwired: 1 in]
            n567 = Not Equal?(x=w1267, y=w1268) -> (x != y?=w1266:bool)
            n568 = case shown="False" w1266 {
              tunnel: ["" ("State with Arguments") w1276] -> w1270
              tunnel: "温控开关 2" -> [_ w1275]
              frame False {
              }
              frame True {
                n569 = call "Convert Data To API String Arguments.vim"("Data"=w1275) -> ("API String"=w1278:string)  [unwired: 7 in, 1 out]
                n570 = call <vilib>:"Build State String with Arguments__JKI_lib_State_Machine.vi"("Arguments (\"\")"=w1278, "State"="Action: Power Output 2" ("State(s) in Front (\"\")")) -> ("State with Arguments"=w1276:string)  [unwired: 4 in]
              }
            }
            n571 = call <vilib>:"Add State(s) to Queue__JKI_lib_State_Machine.vi"("State(s) in Front (\"\")"=w1270, "State(s) in (\"\")"=w1272) -> ("States Out"=w1271:string)  [unwired: 13 in]
          }
          event "温控开关 总": Value Change {
            n572 = event-data() -> ()  [unwired: 1 in, 1 out]
            n573 = call "Convert Data To API String Arguments.vim"("Data"="温控开关 总") -> ("API String"=w1283:string)  [unwired: 7 in, 1 out]
            n574 = call <vilib>:"Build State String with Arguments__JKI_lib_State_Machine.vi"("Arguments (\"\")"=w1283, "State"="Action: Power Output 1" ("State(s) in Front (\"\")")) -> ("State with Arguments"=w1281:string)  [unwired: 4 in]
            n575 = call <vilib>:"Build State String with Arguments__JKI_lib_State_Machine.vi"("Arguments (\"\")"=w1283, "State"="Action: Power Output 2" ("State(s) in Front (\"\")")) -> ("State with Arguments"=w1280:string)  [unwired: 4 in]
            n576 = call <vilib>:"Add State(s) to Queue__JKI_lib_State_Machine.vi"("State(s) in Front (\"\")"=w1281, "State(s) in (\"\")"=w1280) -> ("States Out"=w1279:string)  [unwired: 13 in]
            n577 = call <vilib>:"Add State(s) to Queue__JKI_lib_State_Machine.vi"("State(s) in Front (\"\")"=w1279, "State(s) in (\"\")"=w1287) -> ("States Out"=w1286:string)  [unwired: 13 in]
          }
          event "温控温度 1": Value Change {
            n578 = event-data() -> ("OldVal"=w1295:dbl, "NewVal"=w1294:dbl)  [unwired: 1 in, 1 out]
            n579 = Not Equal?(x=w1295, y=w1294) -> (x != y?=w1292:bool)
            n580 = call "Convert Data To API String Arguments.vim"("Data"="温控温度 1") -> ("API String"=w1297:string)  [unwired: 7 in, 1 out]
            n581 = call <vilib>:"Build State String with Arguments__JKI_lib_State_Machine.vi"("Arguments (\"\")"=w1297, "State"="Action: Change Temp 1" ("State(s) in Front (\"\")")) -> ("State with Arguments"=w1293:string)  [unwired: 4 in]
            n582 = Select(t=w1293, s=w1292, f="") -> (s? t:f=w1290:string)
            n583 = call <vilib>:"Add State(s) to Queue__JKI_lib_State_Machine.vi"("State(s) in Front (\"\")"=w1290, "State(s) in (\"\")"=w1299) -> ("States Out"=w1298:string)  [unwired: 13 in]
          }
          event "温控温度 2": Value Change {
            n584 = event-data() -> ("OldVal"=w1305:dbl, "NewVal"=w1306:dbl)  [unwired: 1 in, 1 out]
            n585 = Not Equal?(x=w1305, y=w1306) -> (x != y?=w1304:bool)
            n586 = call "Convert Data To API String Arguments.vim"("Data"="温控温度 2") -> ("API String"=w1309:string)  [unwired: 7 in, 1 out]
            n587 = call <vilib>:"Build State String with Arguments__JKI_lib_State_Machine.vi"("Arguments (\"\")"=w1309, "State"="Action: Change Temp 2" ("State(s) in Front (\"\")")) -> ("State with Arguments"=w1303:string)  [unwired: 4 in]
            n588 = Select(t=w1303, s=w1304, f="") -> (s? t:f=w1302:string)
            n589 = call <vilib>:"Add State(s) to Queue__JKI_lib_State_Machine.vi"("State(s) in Front (\"\")"=w1302, "State(s) in (\"\")"=w1311) -> ("States Out"=w1310:string)  [unwired: 13 in]
          }
          event "温度": Value Change {
            n590 = event-data() -> ()  [unwired: 1 in, 1 out]
            n591 = Select(t="温控温度 A", s="温度", f="温控温度 B") -> (s? t:f=w1315:dbl)
            n592 = case shown="True" "通道" {
              tunnel: w1315 -> [w1321 w1322]
              frame False {
                n593 = property on="温控温度 2" class="DigNum (严格)"("Val(Sgnl)"=w1321) -> ()  [unwired: 2 in, 2 out]
              }
              frame True {
                n594 = property on="温控温度 1" class="DigNum (严格)"("Val(Sgnl)"=w1322) -> ()  [unwired: 2 in, 2 out]
              }
            }
            n595 = call <vilib>:"Add State(s) to Queue__JKI_lib_State_Machine.vi"("State(s) in (\"\")"=w1313) -> ("States Out"=w1314:string)  [unwired: 14 in]
          }
          event "TC1", "TC2": Autoscale Range Change {
            n596 = event-data() -> ()  [unwired: 1 in, 1 out]
            n597 = call <vilib>:"Add State(s) to Queue__jki_lib_state_machine.vi"("State(s) in Front (\"\")"="UI: Auto Range Change" ("State(s) in Front (\"\")"), "State(s) in (\"\")"=w1324) -> ("States Out"=w1325:string)  [unwired: 13 in]
          }
          event "上限 1", "下限 1", "上限 2", "下限 2": Value Change {
            n598 = event-data() -> ()  [unwired: 1 in, 1 out]
            n599 = call <vilib>:"Add State(s) to Queue__JKI_lib_State_Machine.vi"("State(s) in Front (\"\")"="UI: Gragh Range" ("State(s) in Front (\"\")"), "State(s) in (\"\")"=w1328) -> ("States Out"=w1329:string)  [unwired: 13 in]
          }
          event "电源切换 1": Value Change {
            n600 = event-data() -> ()  [unwired: 1 in, 1 out]
            n601 = call "Convert Data To API String Arguments.vim"("Data"="电源切换 1") -> ("API String"=w1334:string)  [unwired: 7 in, 1 out]
            n602 = call <vilib>:"Build State String with Arguments__JKI_lib_State_Machine.vi"("Arguments (\"\")"=w1334, "State"="Action: Power Switch 1") -> ("State with Arguments"=w1332:string)  [unwired: 4 in]
            n603 = call <vilib>:"Add State(s) to Queue__JKI_lib_State_Machine.vi"("State(s) in Front (\"\")"=w1332, "State(s) in (\"\")"=w1335) -> ("States Out"=w1336:string)  [unwired: 13 in]
          }
          event "电源切换 2": Value Change {
            n604 = event-data() -> ()  [unwired: 1 in, 1 out]
            n605 = call "Convert Data To API String Arguments.vim"("Data"="电源切换 2") -> ("API String"=w1341:string)  [unwired: 7 in, 1 out]
            n606 = call <vilib>:"Build State String with Arguments__JKI_lib_State_Machine.vi"("Arguments (\"\")"=w1341, "State"="Action: Power Switch 2") -> ("State with Arguments"=w1339:string)  [unwired: 4 in]
            n607 = call <vilib>:"Add State(s) to Queue__JKI_lib_State_Machine.vi"("State(s) in Front (\"\")"=w1339, "State(s) in (\"\")"=w1342) -> ("States Out"=w1343:string)  [unwired: 13 in]
          }
          event "Fast Mode": Value Change {
            n608 = event-data() -> ()  [unwired: 1 in, 1 out]
            n609 = call "Convert Data To API String Arguments.vim"("Data"="Fast Mode") -> ("API String"=w1346:string)  [unwired: 7 in, 1 out]
            n610 = call <vilib>:"Build State String with Arguments__JKI_lib_State_Machine.vi"("Arguments (\"\")"=w1346, "State"="Acq: Fast Mode") -> ("State with Arguments"=w1347:string)  [unwired: 4 in]
            n611 = call <vilib>:"Add State(s) to Queue__JKI_lib_State_Machine.vi"("State(s) in Front (\"\")"=w1347, "State(s) in (\"\")"=w1349) -> ("States Out"=w1350:string)  [unwired: 13 in]
          }
          event "采集间隔": Value Change {
            n612 = event-data() -> ()  [unwired: 1 in, 1 out]
            n613 = call "Convert Data To API String Arguments.vim"("Data"="采集间隔") -> ("API String"=w1353:string)  [unwired: 7 in, 1 out]
            n614 = call <vilib>:"Build State String with Arguments__JKI_lib_State_Machine.vi"("Arguments (\"\")"=w1353, "State"="Acq: Sample Interval") -> ("State with Arguments"=w1354:string)  [unwired: 4 in]
            n615 = call <vilib>:"Add State(s) to Queue__JKI_lib_State_Machine.vi"("State(s) in Front (\"\")"=w1354, "State(s) in (\"\")"=w1356) -> ("States Out"=w1357:string)  [unwired: 13 in]
          }
          event "输出设置 1": Value Change {
            n616 = event-data() -> ("OldVal"=w1375:T4, "NewVal"=w1374:T4)  [unwired: 1 in, 1 out]
            n617 = Not Equal?(x=w1375, y=w1374) -> (x != y?=w1376:cluster{"输出模式":bool, "最大输出电压":bool})
            n618 = Cluster To Array(cluster=w1376) -> (array=w1377:bool[])
            n619 = Boolean Array To Number(Boolean array=w1377) -> (number=w1367:u32)
            n620 = Number To Decimal String(number=w1367) -> (decimal integer string=w1369:string)  [unwired: 1 in]
            n621 = case shown="1" w1367 {
              tunnel: "输出设置 1" -> [_ w1388 w1390]
              tunnel: [_ w1387 w1389] -> w1368
              frame 0, Default {
              }
              frame 1 {
                n622 = Unbundle By Name(w1388) -> ("输出模式"=w1387:enum16{"致冷模式", "加热模式", "双向模式"})
              }
              frame 2 {
                n623 = Unbundle By Name(w1390) -> ("最大输出电压"=w1389:dbl)
              }
            }
            n624 = local read "温控开关 1"() -> (w1361:bool)
            n625 = Number To Fractional String(number=w1368) -> (F-format string=w1366:string)  [unwired: 3 in]
            n626 = Concatenate Strings(w1369, "/" ("字符串"), w1366) -> (w1365:string)
            n627 = case shown="True" w1361 {
              tunnel: [w1379 w1381] -> w1360
              tunnel: [w1379 w1380] -> w1359
              frame False {
                w1379 = "" ("State with Arguments")
              }
              frame True {
                w1382 = "Action: Power Output 1"
                n628 = call "Convert Data To API String Arguments.vim"("Data"=TRUE) -> ("API String"=w1383:string)  [unwired: 7 in, 1 out]
                n629 = call "Convert Data To API String Arguments.vim"("Data"=FALSE) -> ("API String"=w1384:string)  [unwired: 7 in, 1 out]
                n630 = call <vilib>:"Build State String with Arguments__JKI_lib_State_Machine.vi"("Arguments (\"\")"=w1384, "State"=w1382) -> ("State with Arguments"=w1381:string)  [unwired: 4 in]
                n631 = call <vilib>:"Build State String with Arguments__JKI_lib_State_Machine.vi"("Arguments (\"\")"=w1383, "State"=w1382) -> ("State with Arguments"=w1380:string)  [unwired: 4 in]
              }
            }
            n632 = call <vilib>:"Build State String with Arguments__JKI_lib_State_Machine.vi"("Arguments (\"\")"=w1365, "State"="Action: Output Set 1") -> ("State with Arguments"=w1362:string)  [unwired: 4 in]
            n633 = call <vilib>:"Add State(s) to Queue__JKI_lib_State_Machine.vi"("State(s) in Front (\"\")"=w1360, "State(s) in (\"\")"=w1362, "State(s) at Back (\"\")"=w1359) -> ("States Out"=w1363:string)  [unwired: 12 in]
            n634 = call <vilib>:"Add State(s) to Queue__JKI_lib_State_Machine.vi"("State(s) in Front (\"\")"=w1363, "State(s) in (\"\")"=w1372) -> ("States Out"=w1373:string)  [unwired: 13 in]
          }
          event "输出设置 2": Value Change {
            n635 = event-data() -> ("OldVal"=w1407:T4, "NewVal"=w1406:T4)  [unwired: 1 in, 1 out]
            n636 = Not Equal?(x=w1407, y=w1406) -> (x != y?=w1408:cluster{"输出模式":bool, "最大输出电压":bool})
            n637 = Cluster To Array(cluster=w1408) -> (array=w1409:bool[])
            n638 = Boolean Array To Number(Boolean array=w1409) -> (number=w1399:u32)
            n639 = Number To Decimal String(number=w1399) -> (decimal integer string=w1401:string)  [unwired: 1 in]
            n640 = case shown="1" w1399 {
              tunnel: "输出设置 2" -> [_ w1420 w1422]
              tunnel: [_ w1419 w1421] -> w1400
              frame 0, Default {
              }
              frame 1 {
                n641 = Unbundle By Name(w1420) -> ("输出模式"=w1419:enum16{"致冷模式", "加热模式", "双向模式"})
              }
              frame 2 {
                n642 = Unbundle By Name(w1422) -> ("最大输出电压"=w1421:dbl)
              }
            }
            n643 = Number To Fractional String(number=w1400) -> (F-format string=w1398:string)  [unwired: 3 in]
            n644 = local read "温控开关 2"() -> (w1391:bool)
            n645 = Concatenate Strings(w1401, "/" ("字符串"), w1398) -> (w1397:string)
            n646 = call <vilib>:"Build State String with Arguments__JKI_lib_State_Machine.vi"("Arguments (\"\")"=w1397, "State"="Action: Output Set 2") -> ("State with Arguments"=w1393:string)  [unwired: 4 in]
            n647 = case shown="True" w1391 {
              tunnel: [w1411 w1413] -> w1395
              tunnel: [w1411 w1412] -> w1394
              frame False {
                w1411 = "" ("State with Arguments")
              }
              frame True {
                w1414 = "Action: Power Output 2"
                n648 = call "Convert Data To API String Arguments.vim"("Data"=TRUE) -> ("API String"=w1415:string)  [unwired: 7 in, 1 out]
                n649 = call "Convert Data To API String Arguments.vim"("Data"=FALSE) -> ("API String"=w1416:string)  [unwired: 7 in, 1 out]
                n650 = call <vilib>:"Build State String with Arguments__JKI_lib_State_Machine.vi"("Arguments (\"\")"=w1416, "State"=w1414) -> ("State with Arguments"=w1413:string)  [unwired: 4 in]
                n651 = call <vilib>:"Build State String with Arguments__JKI_lib_State_Machine.vi"("Arguments (\"\")"=w1415, "State"=w1414) -> ("State with Arguments"=w1412:string)  [unwired: 4 in]
              }
            }
            n652 = call <vilib>:"Add State(s) to Queue__JKI_lib_State_Machine.vi"("State(s) in Front (\"\")"=w1395, "State(s) in (\"\")"=w1393, "State(s) at Back (\"\")"=w1394) -> ("States Out"=w1392:string)  [unwired: 12 in]
            n653 = call <vilib>:"Add State(s) to Queue__JKI_lib_State_Machine.vi"("State(s) in Front (\"\")"=w1392, "State(s) in (\"\")"=w1404) -> ("States Out"=w1405:string)  [unwired: 13 in]
          }
          event "PID 1": Value Change {
            n654 = event-data() -> ("OldVal"=w1430:T5, "NewVal"=w1429:T5)  [unwired: 1 in, 4 out]
            n655 = Not Equal?(x=w1430, y=w1429) -> (x != y?=w1437:T24)
            n656 = Cluster To Array(cluster=w1437) -> (array=w1436:bool[])
            n657 = Boolean Array To Number(Boolean array=w1436) -> (number=w1435:u32)
            n658 = case shown="1" w1435 {
              tunnel: "PID 1" -> [_ w1441 w1443 w1445 w1447 w1449 w1451]
              tunnel: [0.0 ("PID控制间隔") w1440 w1442 w1444 w1446 w1448 w1450] -> w1434
              frame 0, Default {
              }
              frame 1 {
                n659 = Unbundle By Name(w1441) -> ("PID类型"=w1440:enum16{"P", "PI", "PID"})
              }
              frame 2 {
                n660 = Unbundle By Name(w1443) -> ("P"=w1442:dbl)
              }
              frame 4 {
                n661 = Unbundle By Name(w1445) -> ("I"=w1444:dbl)
              }
              frame 8 {
                n662 = Unbundle By Name(w1447) -> ("D"=w1446:dbl)
              }
              frame 16 {
                n663 = Unbundle By Name(w1449) -> ("PID控制间隔"=w1448:dbl)
              }
              frame 32 {
                n664 = Unbundle By Name(w1451) -> ("PID计算方法"=w1450:enum16{"位置式", "增量式", "最大正向输出", "最大负向输出"})
              }
            }
            n665 = Number To Decimal String(number=w1435) -> (decimal integer string=w1433:string)  [unwired: 1 in]
            n666 = Number To Fractional String(number=w1434) -> (F-format string=w1432:string)  [unwired: 3 in]
            n667 = Concatenate Strings(w1433, "/" ("字符串"), w1432) -> (w1425:string)
            n668 = call <vilib>:"Build State String with Arguments__JKI_lib_State_Machine.vi"("Arguments (\"\")"=w1425, "State"="Action: PID Set 1") -> ("State with Arguments"=w1424:string)  [unwired: 4 in]
            n669 = call <vilib>:"Add State(s) to Queue__JKI_lib_State_Machine.vi"("State(s) in Front (\"\")"=w1424, "State(s) in (\"\")"=w1427) -> ("States Out"=w1428:string)  [unwired: 13 in]
          }
          event "PID 2": Value Change {
            n670 = event-data() -> ("OldVal"=w1459:T5, "NewVal"=w1458:T5)  [unwired: 1 in, 4 out]
            n671 = Not Equal?(x=w1459, y=w1458) -> (x != y?=w1466:T24)
            n672 = Cluster To Array(cluster=w1466) -> (array=w1465:bool[])
            n673 = Boolean Array To Number(Boolean array=w1465) -> (number=w1464:u32)
            n674 = case shown="1" w1464 {
              tunnel: "PID 2" -> [_ w1470 w1472 w1474 w1476 w1478 w1480]
              tunnel: [0.0 ("PID控制间隔") w1469 w1471 w1473 w1475 w1477 w1479] -> w1463
              frame 0, Default {
              }
              frame 1 {
                n675 = Unbundle By Name(w1470) -> ("PID类型"=w1469:enum16{"P", "PI", "PID"})
              }
              frame 2 {
                n676 = Unbundle By Name(w1472) -> ("P"=w1471:dbl)
              }
              frame 4 {
                n677 = Unbundle By Name(w1474) -> ("I"=w1473:dbl)
              }
              frame 8 {
                n678 = Unbundle By Name(w1476) -> ("D"=w1475:dbl)
              }
              frame 16 {
                n679 = Unbundle By Name(w1478) -> ("PID控制间隔"=w1477:dbl)
              }
              frame 32 {
                n680 = Unbundle By Name(w1480) -> ("PID计算方法"=w1479:enum16{"位置式", "增量式", "最大正向输出", "最大负向输出"})
              }
            }
            n681 = Number To Decimal String(number=w1464) -> (decimal integer string=w1462:string)  [unwired: 1 in]
            n682 = Number To Fractional String(number=w1463) -> (F-format string=w1461:string)  [unwired: 3 in]
            n683 = Concatenate Strings(w1462, "/" ("字符串"), w1461) -> (w1454:string)
            n684 = call <vilib>:"Build State String with Arguments__JKI_lib_State_Machine.vi"("Arguments (\"\")"=w1454, "State"="Action: PID Set 2") -> ("State with Arguments"=w1453:string)  [unwired: 4 in]
            n685 = call <vilib>:"Add State(s) to Queue__JKI_lib_State_Machine.vi"("State(s) in Front (\"\")"=w1453, "State(s) in (\"\")"=w1456) -> ("States Out"=w1457:string)  [unwired: 13 in]
          }
          event "过温 1": Value Change {
            n686 = event-data() -> ("OldVal"=w1488:T6, "NewVal"=w1487:T6)  [unwired: 1 in, 4 out]
            n687 = Not Equal?(x=w1488, y=w1487) -> (x != y?=w1495:T25)
            n688 = Cluster To Array(cluster=w1495) -> (array=w1494:bool[])
            n689 = Boolean Array To Number(Boolean array=w1494) -> (number=w1493:u32)
            n690 = case shown="0, 默认" w1493 {
              tunnel: "过温 1" -> [_ w1500 w1502 w1504 w1506 w1508 w1510]
              tunnel: [0.0 ("温度限速") w1498 w1501 w1503 w1505 w1507 w1509] -> w1492
              frame 0, Default {
              }
              frame 1 {
                n691 = Unbundle By Name(w1500) -> ("过温保护开关"=w1499:bool)
                n692 = Boolean To (0,1)(Boolean=w1499) -> (0, 1=w1498:i16)
              }
              frame 2 {
                n693 = Unbundle By Name(w1502) -> ("过温保护低阈值"=w1501:dbl)
              }
              frame 4 {
                n694 = Unbundle By Name(w1504) -> ("过温保护高阈值"=w1503:dbl)
              }
              frame 8 {
                n695 = Unbundle By Name(w1506) -> ("最低设定温度"=w1505:dbl)
              }
              frame 16 {
                n696 = Unbundle By Name(w1508) -> ("最高设定温度"=w1507:dbl)
              }
              frame 32 {
                n697 = Unbundle By Name(w1510) -> ("温度限速"=w1509:dbl)
              }
            }
            n698 = Number To Decimal String(number=w1493) -> (decimal integer string=w1491:string)  [unwired: 1 in]
            n699 = Number To Fractional String(number=w1492) -> (F-format string=w1490:string)  [unwired: 3 in]
            n700 = Concatenate Strings(w1491, "/" ("字符串"), w1490) -> (w1483:string)
            n701 = call <vilib>:"Build State String with Arguments__JKI_lib_State_Machine.vi"("Arguments (\"\")"=w1483, "State"="Action: OTP Set 1") -> ("State with Arguments"=w1482:string)  [unwired: 4 in]
            n702 = call <vilib>:"Add State(s) to Queue__JKI_lib_State_Machine.vi"("State(s) in Front (\"\")"=w1482, "State(s) in (\"\")"=w1485) -> ("States Out"=w1486:string)  [unwired: 13 in]
          }
          event "过温 2": Value Change {
            n703 = event-data() -> ("OldVal"=w1518:T6, "NewVal"=w1517:T6)  [unwired: 1 in, 4 out]
            n704 = Not Equal?(x=w1518, y=w1517) -> (x != y?=w1525:T25)
            n705 = Cluster To Array(cluster=w1525) -> (array=w1524:bool[])
            n706 = Boolean Array To Number(Boolean array=w1524) -> (number=w1523:u32)
            n707 = case shown="0, 默认" w1523 {
              tunnel: "过温 2" -> [_ w1530 w1532 w1534 w1536 w1538 w1540]
              tunnel: [0.0 ("温度限速") w1528 w1531 w1533 w1535 w1537 w1539] -> w1522
              frame 0, Default {
              }
              frame 1 {
                n708 = Unbundle By Name(w1530) -> ("过温保护开关"=w1529:bool)
                n709 = Boolean To (0,1)(Boolean=w1529) -> (0, 1=w1528:i16)
              }
              frame 2 {
                n710 = Unbundle By Name(w1532) -> ("过温保护低阈值"=w1531:dbl)
              }
              frame 4 {
                n711 = Unbundle By Name(w1534) -> ("过温保护高阈值"=w1533:dbl)
              }
              frame 8 {
                n712 = Unbundle By Name(w1536) -> ("最低设定温度"=w1535:dbl)
              }
              frame 16 {
                n713 = Unbundle By Name(w1538) -> ("最高设定温度"=w1537:dbl)
              }
              frame 32 {
                n714 = Unbundle By Name(w1540) -> ("温度限速"=w1539:dbl)
              }
            }
            n715 = Number To Decimal String(number=w1523) -> (decimal integer string=w1521:string)  [unwired: 1 in]
            n716 = Number To Fractional String(number=w1522) -> (F-format string=w1520:string)  [unwired: 3 in]
            n717 = Concatenate Strings(w1521, "/" ("字符串"), w1520) -> (w1513:string)
            n718 = call <vilib>:"Build State String with Arguments__JKI_lib_State_Machine.vi"("Arguments (\"\")"=w1513, "State"="Action: OTP Set 2") -> ("State with Arguments"=w1512:string)  [unwired: 4 in]
            n719 = call <vilib>:"Add State(s) to Queue__JKI_lib_State_Machine.vi"("State(s) in Front (\"\")"=w1512, "State(s) in (\"\")"=w1515) -> ("States Out"=w1516:string)  [unwired: 13 in]
          }
          event "过压/过流 1": Value Change {
            n720 = event-data() -> ("OldVal"=w1552:cluster{"过压保护阈值":dbl, "过流保护阈值":dbl}, "NewVal"=w1551:cluster{"过压保护阈值":dbl, "过流保护阈值":dbl})  [unwired: 1 in]
            n721 = Not Equal?(x=w1552, y=w1551) -> (x != y?=w1559:cluster{"过压保护阈值":bool, "过流保护阈值":bool})
            n722 = Cluster To Array(cluster=w1559) -> (array=w1558:bool[])
            n723 = Boolean Array To Number(Boolean array=w1558) -> (number=w1557:u32)
            n724 = case shown="1" w1557 {
              tunnel: "过压/过流 1" -> [_ w1571 w1573]
              tunnel: [0.0 ("过流保护阈值") w1570 w1572] -> w1556
              frame 0, Default {
              }
              frame 1 {
                n725 = Unbundle By Name(w1571) -> ("过压保护阈值"=w1570:dbl)
              }
              frame 2 {
                n726 = Unbundle By Name(w1573) -> ("过流保护阈值"=w1572:dbl)
              }
            }
            n727 = Number To Decimal String(number=w1557) -> (decimal integer string=w1555:string)  [unwired: 1 in]
            n728 = local read "温控开关 1"() -> (w1541:bool)
            n729 = Number To Fractional String(number=w1556) -> (F-format string=w1554:string)  [unwired: 3 in]
            n730 = Concatenate Strings(w1555, "/" ("字符串"), w1554) -> (w1547:string)
            n731 = case shown="True" w1541 {
              tunnel: [w1561 w1563] -> w1545
              tunnel: [w1561 w1562] -> w1544
              frame False {
                w1561 = "" ("State with Arguments")
              }
              frame True {
                w1564 = "Action: Power Output 1"
                n732 = call "Convert Data To API String Arguments.vim"("Data"=TRUE) -> ("API String"=w1565:string)  [unwired: 7 in, 1 out]
                n733 = call "Convert Data To API String Arguments.vim"("Data"=FALSE) -> ("API String"=w1566:string)  [unwired: 7 in, 1 out]
                n734 = call <vilib>:"Build State String with Arguments__JKI_lib_State_Machine.vi"("Arguments (\"\")"=w1566, "State"=w1564) -> ("State with Arguments"=w1563:string)  [unwired: 4 in]
                n735 = call <vilib>:"Build State String with Arguments__JKI_lib_State_Machine.vi"("Arguments (\"\")"=w1565, "State"=w1564) -> ("State with Arguments"=w1562:string)  [unwired: 4 in]
              }
            }
            n736 = call <vilib>:"Build State String with Arguments__JKI_lib_State_Machine.vi"("Arguments (\"\")"=w1547, "State"="Action: OVP Set 1") -> ("State with Arguments"=w1543:string)  [unwired: 4 in]
            n737 = call <vilib>:"Add State(s) to Queue__JKI_lib_State_Machine.vi"("State(s) in Front (\"\")"=w1545, "State(s) in (\"\")"=w1543, "State(s) at Back (\"\")"=w1544) -> ("States Out"=w1542:string)  [unwired: 12 in]
            n738 = call <vilib>:"Add State(s) to Queue__JKI_lib_State_Machine.vi"("State(s) in Front (\"\")"=w1542, "State(s) in (\"\")"=w1549) -> ("States Out"=w1550:string)  [unwired: 13 in]
          }
          event "过压/过流 2": Value Change {
            n739 = event-data() -> ("OldVal"=w1585:cluster{"过压保护阈值":dbl, "过流保护阈值":dbl}, "NewVal"=w1584:cluster{"过压保护阈值":dbl, "过流保护阈值":dbl})  [unwired: 1 in]
            n740 = Not Equal?(x=w1585, y=w1584) -> (x != y?=w1592:cluster{"过压保护阈值":bool, "过流保护阈值":bool})
            n741 = Cluster To Array(cluster=w1592) -> (array=w1591:bool[])
            n742 = Boolean Array To Number(Boolean array=w1591) -> (number=w1590:u32)
            n743 = case shown="2" w1590 {
              tunnel: "过压/过流 2" -> [_ w1604 w1606]
              tunnel: [0.0 ("过流保护阈值") w1603 w1605] -> w1589
              frame 0, Default {
              }
              frame 1 {
                n744 = Unbundle By Name(w1604) -> ("过压保护阈值"=w1603:dbl)
              }
              frame 2 {
                n745 = Unbundle By Name(w1606) -> ("过流保护阈值"=w1605:dbl)
              }
            }
            n746 = Number To Decimal String(number=w1590) -> (decimal integer string=w1588:string)  [unwired: 1 in]
            n747 = Number To Fractional String(number=w1589) -> (F-format string=w1587:string)  [unwired: 3 in]
            n748 = local read "温控开关 2"() -> (w1574:bool)
            n749 = Concatenate Strings(w1588, "/" ("字符串"), w1587) -> (w1580:string)
            n750 = call <vilib>:"Build State String with Arguments__JKI_lib_State_Machine.vi"("Arguments (\"\")"=w1580, "State"="Action: OVP Set 2") -> ("State with Arguments"=w1576:string)  [unwired: 4 in]
            n751 = case shown="True" w1574 {
              tunnel: [w1594 w1596] -> w1578
              tunnel: [w1594 w1595] -> w1577
              frame False {
                w1594 = "" ("State with Arguments")
              }
              frame True {
                w1597 = "Action: Power Output 2"
                n752 = call "Convert Data To API String Arguments.vim"("Data"=TRUE) -> ("API String"=w1598:string)  [unwired: 7 in, 1 out]
                n753 = call "Convert Data To API String Arguments.vim"("Data"=FALSE) -> ("API String"=w1599:string)  [unwired: 7 in, 1 out]
                n754 = call <vilib>:"Build State String with Arguments__JKI_lib_State_Machine.vi"("Arguments (\"\")"=w1599, "State"=w1597) -> ("State with Arguments"=w1596:string)  [unwired: 4 in]
                n755 = call <vilib>:"Build State String with Arguments__JKI_lib_State_Machine.vi"("Arguments (\"\")"=w1598, "State"=w1597) -> ("State with Arguments"=w1595:string)  [unwired: 4 in]
              }
            }
            n756 = call <vilib>:"Add State(s) to Queue__JKI_lib_State_Machine.vi"("State(s) in Front (\"\")"=w1578, "State(s) in (\"\")"=w1576, "State(s) at Back (\"\")"=w1577) -> ("States Out"=w1575:string)  [unwired: 12 in]
            n757 = call <vilib>:"Add State(s) to Queue__JKI_lib_State_Machine.vi"("State(s) in Front (\"\")"=w1575, "State(s) in (\"\")"=w1582) -> ("States Out"=w1583:string)  [unwired: 13 in]
          }
          event "温控循环功能": Value Change {
            n758 = event-data() -> ("OldVal"=w1608:bool, "NewVal"=w1609:bool)  [unwired: 1 in, 4 out]
            n759 = Not Equal?(x=w1608, y=w1609) -> (x != y?=w1607:bool)
            n760 = case shown="True" w1607 {
              tunnel: ["" w1617] -> w1611
              tunnel: "温控循环功能" -> [_ w1616]
              frame False {
              }
              frame True {
                n761 = Select(t="Repeat: Enable", s=w1616, f="Repeat: Disable") -> (s? t:f=w1617:string)
              }
            }
            n762 = call <vilib>:"Add State(s) to Queue__JKI_lib_State_Machine.vi"("State(s) in Front (\"\")"=w1611, "State(s) in (\"\")"=w1612) -> ("States Out"=w1613:string)  [unwired: 13 in]
          }
        }
      }
      frame "Exit" {
        n763 = Unregister For Events(event registration refnum=w1622) -> (error out=w1621:errorcluster)  [unwired: 1 in]
        n764 = call <vilib>:"Clear Errors.vi"("error in (no error)"=w1621) -> ()  [unwired: 5 in, 2 out]
      }
    }
  }
  n765 = call <userlib>:"CSM - Sync Configuration Variables to File.vi"("All Temp Variable to Default Ini(F)"=TRUE, "error in (no error)"=w4) -> ()  [unwired: 7 in, 1 out]
